vi "Beta.vi"() -> ()   [LabVIEW 2019]
uses:
  Classes/Settings/ObjectSettings/ObjectSettings.lvclass/ObjectSettings.ctl
  <vilib>/Utility/miscctls.llb/LVPositionTypeDef.ctl
  Classes/Parse/ParseVectorFile/ParseVectorFile.lvclass
  C:/Program Files/National Instruments/LabVIEW 2019/vi.lib/JKI/JKI SMO/SMO/SMO.lvclass
  Classes/Settings/Setting Database/Setting Database.lvclass
  Classes/Tool/Tool Data/Tool Data/Tool Data.lvclass
  Classes/Subpanel/Manager/Subpanel.Edit.lvclass
  C:/Users/Albro/Documents/GitHub/AFM-Lithography/lvsrc/Classes/Subpanel/Subpanel.lvclass
  Classes/Render/BigMAQ/BigMAQ.lvclass
  Classes/Selector/Selector.lvclass
  subVIs/AFM API/AFM_Driver_Manager/AFM_Driver_Manager.lvclass
  <userlib>/Levylab/Configuration/Configuration.lvclass
  Classes/Settings/Setting Database/Typedefs/PublicEvents--Setting Database.RectanglesUpdated.ctl
  Classes/Settings/Rectangle Settings/Rectangle Settings.lvclass
  C:/Users/Albro/Documents/GitHub/AFM-Lithography/lvsrc/Classes/Settings/ObjectSettings/ObjectSettings.lvclass
  Classes/Settings/Setting Database/Typedefs/PublicEvents--Setting Database.PathsUpdated.ctl
  Classes/Settings/Path Settings/Path Settings.lvclass
  Classes/Settings/Setting Database/Typedefs/PublicEvents--Setting Database.FunnelsUpdated.ctl
  Classes/Settings/Funnel Settings/Funnel Settings.lvclass
  Classes/Settings/Setting Database/Typedefs/PublicEvents--Setting Database.DotsUpdated.ctl
  Classes/Settings/Dot Settings/Dot Settings.lvclass
  Classes/Parse/ParsePaths/Path.lvclass
  Classes/Parse/Rectangle/Rectangle.lvclass
  Classes/Parse/Image/SVGImage.lvclass
  Classes/Parse/Dot/Dot.lvclass
  <userlib>/Levylab/Relay Box/Typedefs/Resistor--enum.ctl
  Classes/Render/Inset/Inset.lvclass
  Classes/Log/Log.Litho/Log.Litho.lvclass
  Classes/Settings/Setting Database/Typedefs/PrivateEvents--Setting Database.Add To Group.ctl
  Classes/Settings/Setting Database/Typedefs/PrivateEvents--Setting Database.Create New Group.ctl
  Classes/Settings/Setting Database/Typedefs/PrivateEvents--Setting Database.Refresh.ctl
  Classes/Tool/Tool Data/Tool Data/Typedefs/PrivateEvents--Tool Data.Update Objects.ctl
  Classes/Parse/Image/SVGImage.lvclass/SVGImage.ctl
  Classes/Archiver/ArchiveData.ctl
  Controls/Configuration.ctl
  a998b7c0-e198-41fb-897a-9ce541eca358.vi
  <vilib>/Platform/browser.llb/Open URL in Default Browser (string).vi
  <vilib>/Utility/sysdir.llb/Get System Directory.vi
  Classes/Tool/Tool Path/Tool Path.lvclass
  Classes/Tool/Tool Funnel/Tool Funnel.lvclass
  Classes/Tool/Tool Rectangle/Tool Rectangle.lvclass
  Classes/Tool/Tool Dot/Tool Dots.lvclass
  <userlib>/Levylab/Relay Box/Relay-Box.lvclass
  Classes/Subpanel/Subpanel.lvclass
  <vilib>/JKI/JKI SMO/SMO/SMO.lvclass
  Classes/Settings/ObjectSettings/ObjectSettings.lvclass
  Classes/Identity/Identifier.lvclass
  Classes/Archiver/Archivist.lvclass
panel:
  in  "Tab Selectors":T1(radio)
  out "Zoom":string
  in  "Zoom Type":enum32{"Zoom In", "Zoom Out"}(radio)
  in  "Zoom to Fit":bool
  out "Render":T2(plugin-control)
  out "version":string
  out "Ready?":bool
  out "Estimated Time":string
  in  "Run":bool
  in  "Refresh Button":bool
  in  "Done":bool
  in  "Help":bool
  in  "Abort":bool
  in  "Settings":T3(tab)
  in  "Unarchive":bool
  in  "Archive":bool
  out "Status":string
  in  "Inkscape File (.svg)":path caption="Path"
  in  "Background Image":path caption="Path"
  in  "MCLB":i32(listbox) caption="Multicolumn Listbox 2"
  in  "Type:":u16(ring) caption="Ring" items=["Asylum"]
  in  "CopyRender":bool caption="Save"
  in  "Normal Save Path":path caption="Path"
  in  "Save Render":bool caption="Save"
  out "Slow Alert":bool
  in  "Pixellate?":bool
  out "Sizes Match?":bool
  in  "Overwrite?":bool
  in  "Autosave?":bool
  in  "Autosave Path":path caption="Path"
  out "Image Filename":string
  in  "Image Data Range":cluster{sgl, sgl}(slide)={100.0, 0.0} scale=0.0..100.0
  in  "Data Channel":u32 caption="Numeric" max=3
  in  "Inset Editor":bool
  in  "Voltage Color Scale":dbl caption="Numeric 2"
  in  "Hide Labels?":bool
  # "AFM Lithography"
  # "Patterns"
  # "Object Settings"
  # "Atomic Force Microscope Settings"
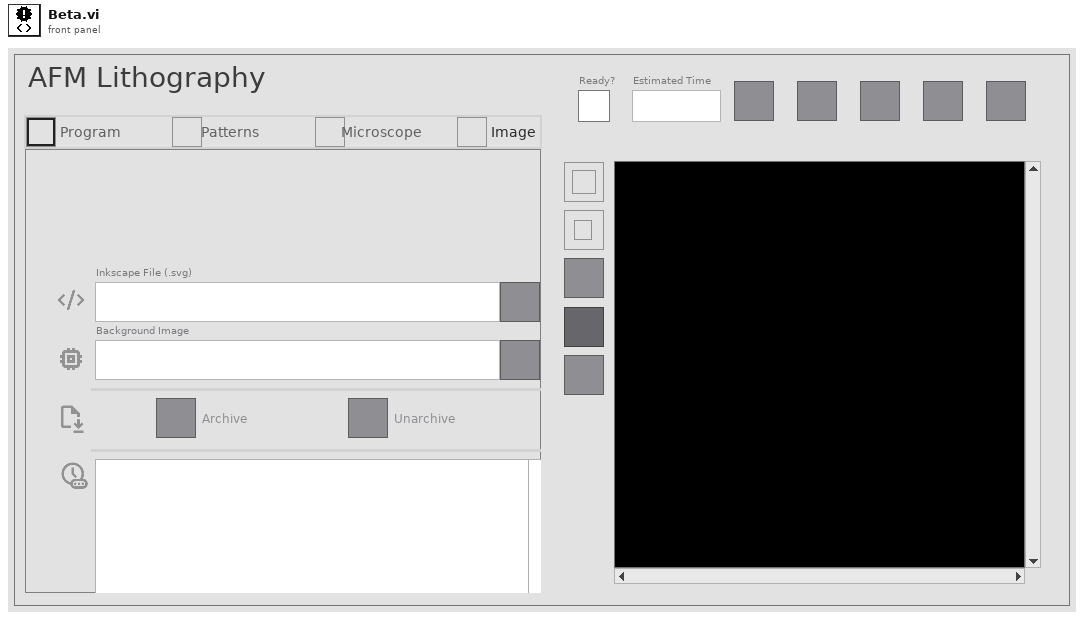
[diagram p1: front panel]
types:
  T1 = enum32{"Home", "Patterns", "Microscope", "Image"}
  T2 = typedef "IMAQ Image.ctl" = refnum<image>
  T3 = enum32{"Program Settings", "Patterns and Writing", "AFM Settings", "Image Settings"}
  T4 = cluster{"Groups":string[], "Enable Items":bool[]}
  T5 = typedef "LVPositionTypeDef.ctl" = cluster{"Left":i32, "Top":i32}
  T6 = cluster{"Point":T5, "Button":u16, "PlatMods":cluster{"Shift":bool, "Ctrl":bool, "Alt":bool, "Cmd":bool, "Opt":bool}}
  T7 = enum32{"Invalid", "Standard", "Closed", "Hidden", "Minimized", "Maximized"}
  T8 = enum32{"invalid app kind", "Development System", "Run Time System", "Student Edition", "Embedded LabVIEW", "Evaluation", "Custom"}
  T9 = cluster{"Background.Range":cluster{sgl, sgl}, "Background.Page":i32}
  T10 = enum8{"Enabled", "Disabled", "Disabled and Grayed Out"}
  T11 = cluster{"Pattern":string, "Pattern Label":string, "Prompt":string}
  T12 = cluster{"paths":string[], "funnels":string[], "rects":string[], "dots":string[]}
  T13 = typedef "Setting Database.lvclass/PrivateEvents--Setting Database.Add To Group.ctl" = cluster{"Name":string, "Group":string}
  T14 = typedef "Setting Database.lvclass/PrivateEvents--Setting Database.Create New Group.ctl" = cluster{"Name":string, "Group":string}
  T15 = typedef "Setting Database.lvclass/PrivateEvents--Setting Database.Refresh.ctl" = cluster{"Paths":string[], "Rectangles":string[], "Funnels":string[], "Dots":string[]}
  T16 = cluster{"Paths":refnum<class "Path.lvclass">[], "Rectangles":refnum<class "Rectangle.lvclass">[], "SVGImage":refnum<class "SVGImage.lvclass">, "Dots":refnum<class "Dot.lvclass">[], "Funnels":refnum<class "Path.lvclass">[]}
  T17 = typedef "Tool Data.lvclass/PrivateEvents--Tool Data.Update Objects.ctl" = cluster{"Settings":cluster{"Paths":T18, "Rectangles":T19, "Funnels":T20, "Dots":T21}, "Data":cluster{"Paths":refnum<class "Path.lvclass">[], "Rectangles":refnum<class "Rectangle.lvclass">[], "SVGImage":refnum<class "SVGImage.lvclass">, "Dots":refnum<class "Dot.lvclass">[], "Funnels":refnum<class "Path.lvclass">[]}}
  T18 = typedef "Setting Database.lvclass/PublicEvents--Setting Database.PathsUpdated.ctl" = refnum<class "Path Settings.lvclass">[]
  T19 = typedef "Setting Database.lvclass/PublicEvents--Setting Database.RectanglesUpdated.ctl" = refnum<class "Rectangle Settings.lvclass">[]
  T20 = typedef "Setting Database.lvclass/PublicEvents--Setting Database.FunnelsUpdated.ctl" = refnum<class "Funnel Settings.lvclass">[]
  T21 = typedef "Setting Database.lvclass/PublicEvents--Setting Database.DotsUpdated.ctl" = refnum<class "Dot Settings.lvclass">[]
  T22 = typedef "Archivist.lvclass/ArchiveData.ctl" = cluster{"Settings":cluster{"Paths":T18, "Rectangles":T19, "Funnels":T20, "Dots":T21}, "Data Files":cluster{"svg":path, "afm":path, "jpg":path}, "Input Path":path, "Order":string[]}
  T23 = typedef "Configuration.ctl" = cluster{"Inkscape Path":path, "Background Path":path, "Autosave Render Path":path, "Autosave Render":bool, "Hide Labels":bool, "Normal Render Path":path, "Overwrite":bool}
  T24 = typedef "Relay-Box.lvclass/Resistor--enum.ctl" = enum16{"open", "discharge tip", "0 ohms", "100k ohm", "10M ohm", "1G ohm"}
  T25 = cluster{"Core":cluster{"Current VI Reference":refnum<vi>, "Close Panel on Exit?":bool}, "tooler":refnum<class "Tool Data.lvclass">, "parser":refnum<class "ParseVectorFile.lvclass">, "settings":refnum<class "Setting Database.lvclass">, "selector":refnum<class "Selector.lvclass">, "sbpnl.edit":refnum<class "Subpanel.Edit.lvclass">, "big-maq":refnum<class "BigMAQ.lvclass">, "config":refnum<class "Configuration.lvclass">, "afm_mngr":refnum<class "AFM_Driver_Manager.lvclass">, "Obj Settings":cluster{"Rectangles":T19, "Paths":T18, "Funnels":T20, "Dots":T21}, "Changed Obj":cluster{"Path Changes":cluster{bool, "index of element":i32}[], "Funnel Changes":cluster{bool, "index of element":i32}[], "Rectangle Changes":cluster{bool, "index of element":i32}[], "Dot Changes":cluster{bool, "index of element":i32}[]}, "GUIDs":cluster{"Dots":string[], "Funnels":string[], "Rects":string[], "Paths":string[]}, "Parsed Obj":cluster{"Paths":refnum<class "Path.lvclass">[], "Rectangles":refnum<class "Rectangle.lvclass">[], "Background":refnum<class "SVGImage.lvclass">, "Dots":refnum<class "Dot.lvclass">[], "Funnels":refnum<class "Path.lvclass">[], "Other Images":refnum<class "SVGImage.lvclass">[]}, "Litho":cluster{"Name":string, "Litho":cluster{"X":dbl, "Y":dbl, "Speed":dbl, "Voltage":dbl}[], "Set Resistance":T24, "Meta":variant}[], "root path":path, "UI":cluster{"Hide Labels":bool, "Image Data Range":cluster{sgl, sgl}, "Status":string, "Autosave Path":path, "Autosave?":bool, "Inkscape File (.svg)":path, "Background Image":path, "Page":u32, "Normal Save Path":path, "Overwrite":bool, "Pixellate?":bool}, "inset":refnum<class "Inset.lvclass">, "log":refnum<class "Log.Litho.lvclass">, "Offline Log":string, "Zoom History":cluster{"X":sgl, "Y":sgl}[], "Archive Location":path, "Cancel Archive":bool}
  T26 = typedef "LVPoint32TypeDef.ctl" = cluster{"Horizontal":i32, "Vertical":i32}
  T27 = cluster{"Paths":refnum<class "Tool Path.lvclass">[], "Funnels":refnum<class "Tool Funnel.lvclass">[], "Rectangles":refnum<class "Tool Rectangle.lvclass">[], "Dots":refnum<class "Tool Dots.lvclass">[]}
  T28 = cluster{"Shift":bool, "Ctrl":bool, "Alt":bool, "Cmd":bool, "Opt":bool}
  T29 = cluster{"Hide Labels":bool, "Image Data Range":cluster{sgl, sgl}, "Status":string, "Autosave Path":path, "Autosave?":bool, "Inkscape File (.svg)":path, "Background Image":path, "Page":u32, "Normal Save Path":path, "Overwrite":bool, "Pixellate?":bool}
  T30 = cluster{"Name":string, "Litho":cluster{"X":dbl, "Y":dbl, "Speed":dbl, "Voltage":dbl}[], "Set Resistance":T24, "Meta":variant}[]
  T31 = cluster{"Paths":refnum<class "Path.lvclass">[], "Rectangles":refnum<class "Rectangle.lvclass">[], "Background":refnum<class "SVGImage.lvclass">, "Dots":refnum<class "Dot.lvclass">[], "Funnels":refnum<class "Path.lvclass">[], "Other Images":refnum<class "SVGImage.lvclass">[]}
  T32 = cluster{"Dots":string[], "Funnels":string[], "Rects":string[], "Paths":string[]}
  T33 = cluster{"Path Changes":cluster{bool, "index of element":i32}[], "Funnel Changes":cluster{bool, "index of element":i32}[], "Rectangle Changes":cluster{bool, "index of element":i32}[], "Dot Changes":cluster{bool, "index of element":i32}[]}
  T34 = cluster{"Rectangles":T19, "Paths":T18, "Funnels":T20, "Dots":T21}
  T35 = cluster{"Current VI Reference":refnum<vi>, "Close Panel on Exit?":bool}
  T36 = typedef "AFM_Driver_Manager.lvclass/AFM_Driver_Manager.PublicEvents.ctl" = cluster{"Lithography Done":refnum<user-event>}
  T37 = typedef "Setting Database.lvclass/PublicEvents--Cluster.ctl" = cluster{"NewActivePath":refnum<user-event>, "PathsUpdated":refnum<user-event>, "RectanglesUpdated":refnum<user-event>, "NewActiveRectangle":refnum<user-event>, "NewActiveFunnel":refnum<user-event>, "FunnelsUpdated":refnum<user-event>, "NewActiveDot":refnum<user-event>, "DotsUpdated":refnum<user-event>}
  T38 = typedef "ParseVectorFile.lvclass/PublicEvents--Cluster.ctl" = cluster{"ParsedData":refnum<user-event>}
  T39 = typedef "Tool Data.lvclass/PublicEvents--Cluster.ctl" = cluster{"Objects Updated":refnum<user-event>}
  T40 = typedef "SMO.lvclass/SMOState --Enum.ctl" = enum16{"unknown", "Created", "Started", "Stopped"}
  T41 = typedef "Selector.lvclass/Item.ctl" = cluster{"Name":string, "Group":string, "Enabled":bool}
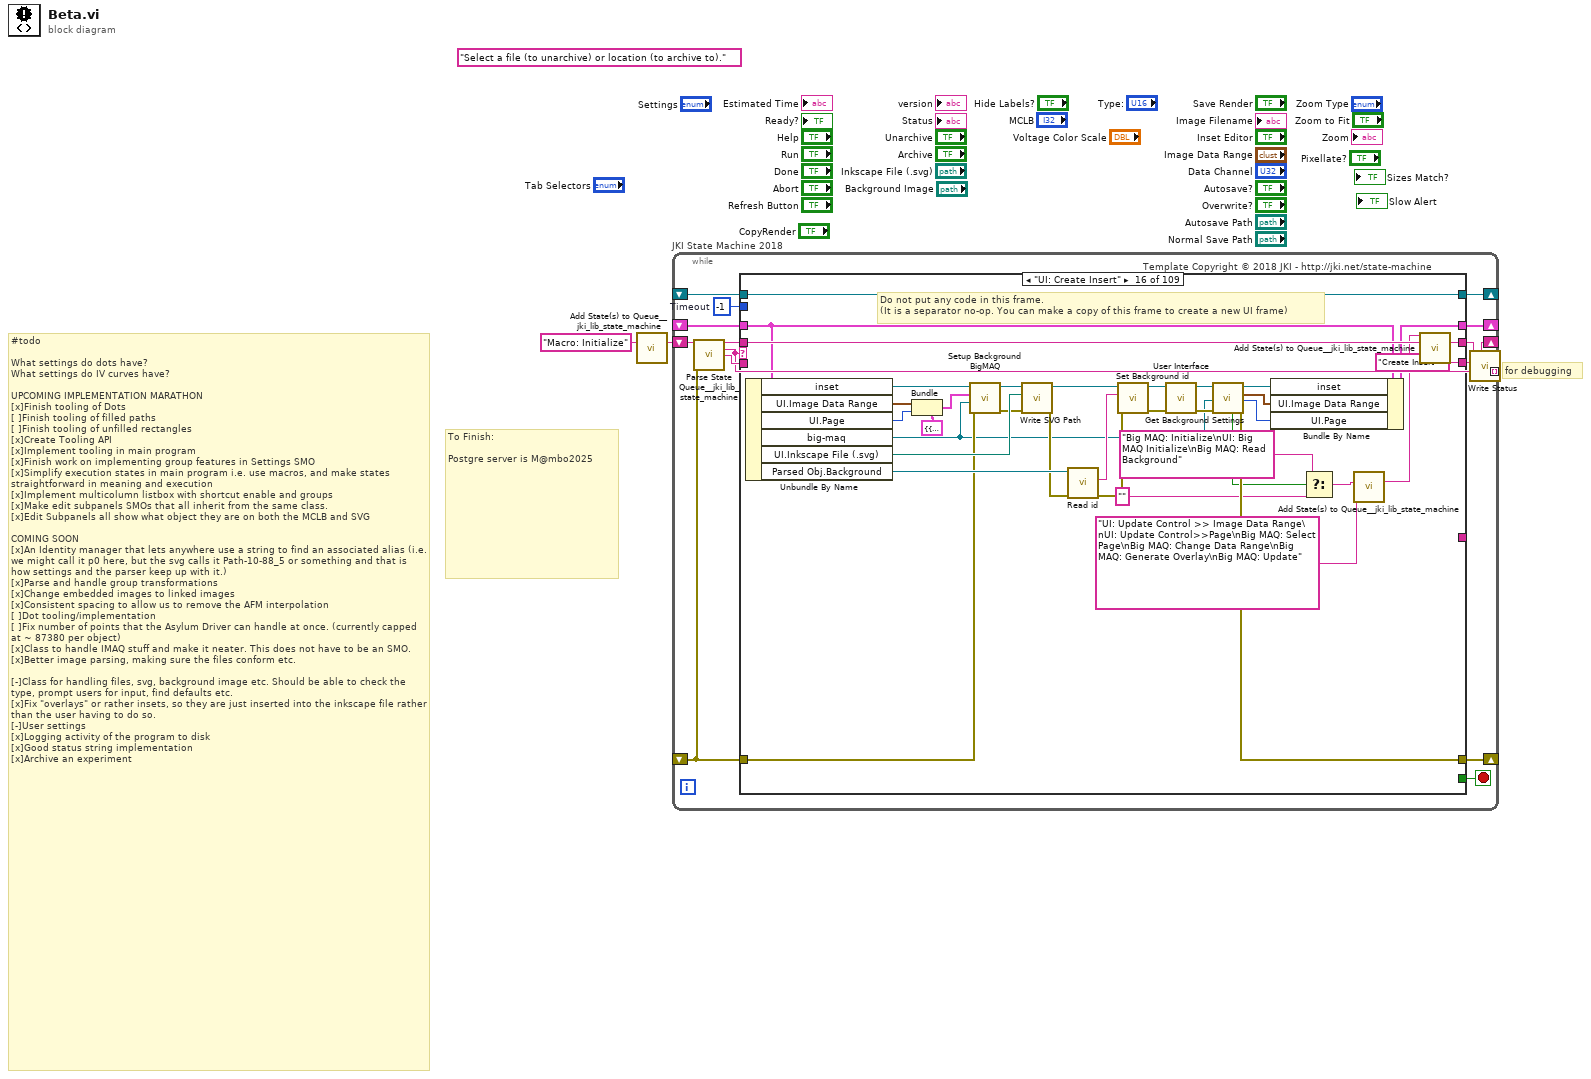
[diagram p0: block diagram]
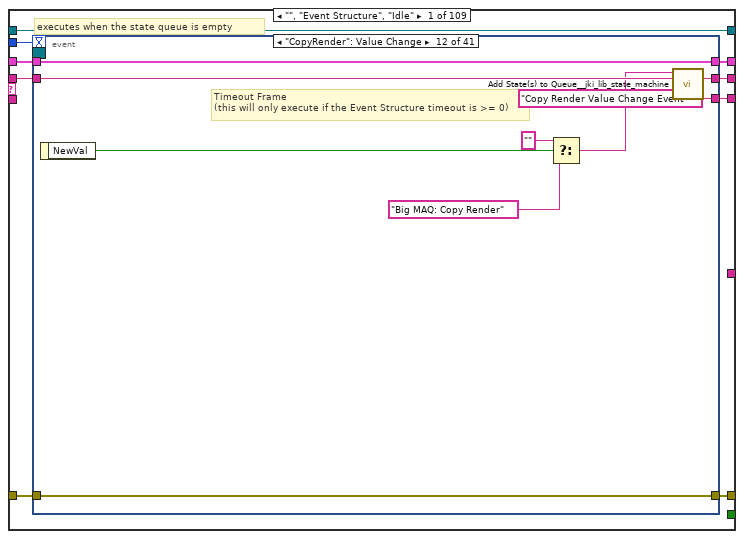
[diagram p2: hidden frame]
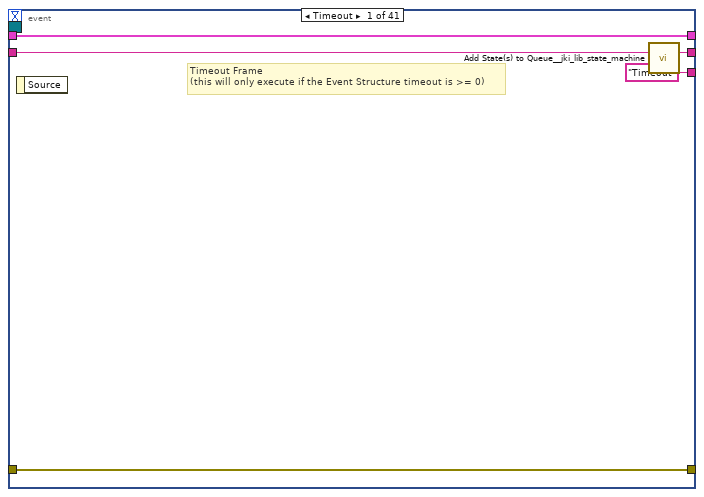
[diagram p3: hidden frame]
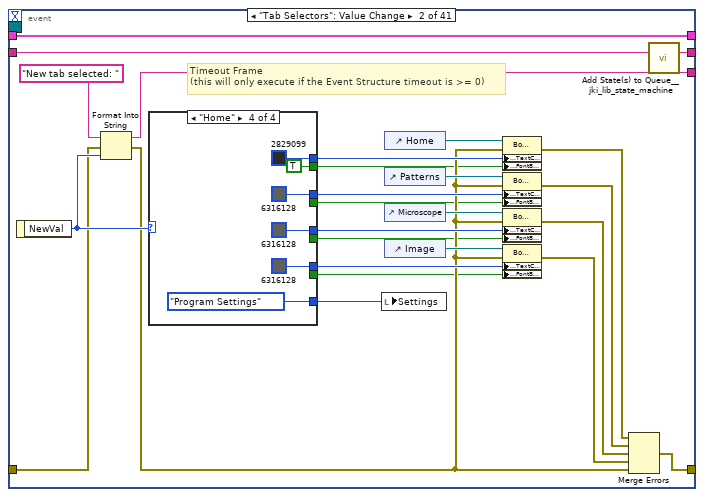
[diagram p4: hidden frame]
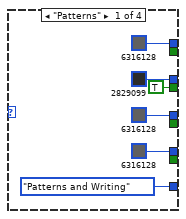
[diagram p5: hidden frame]
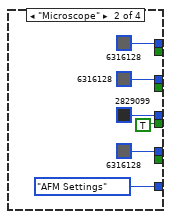
[diagram p6: hidden frame]
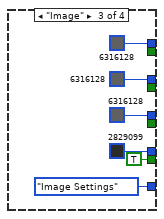
[diagram p7: hidden frame]
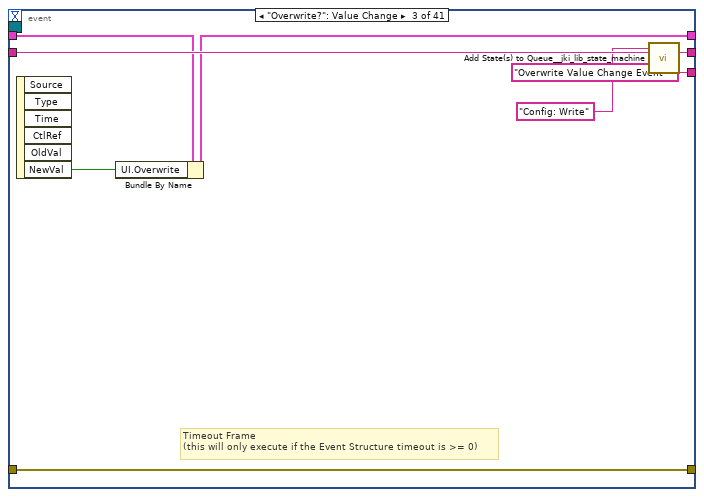
[diagram p8: hidden frame]
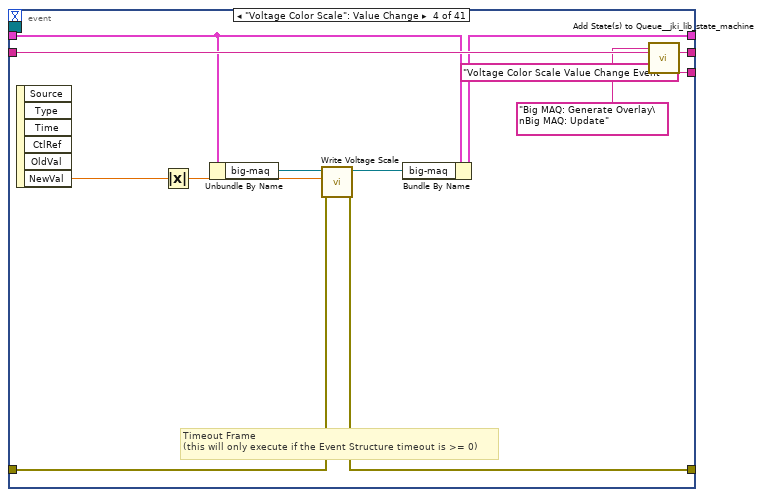
[diagram p9: hidden frame]
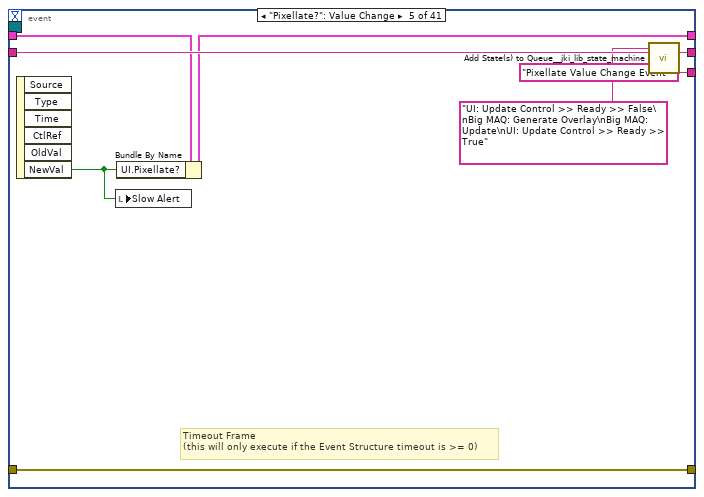
[diagram p10: hidden frame]
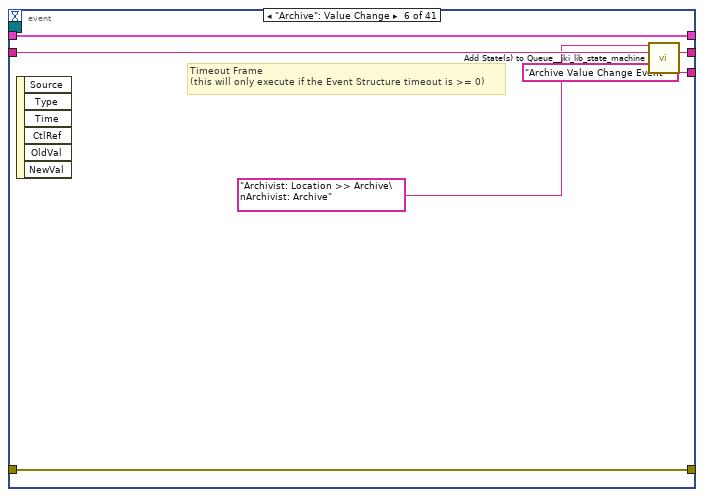
[diagram p11: hidden frame]
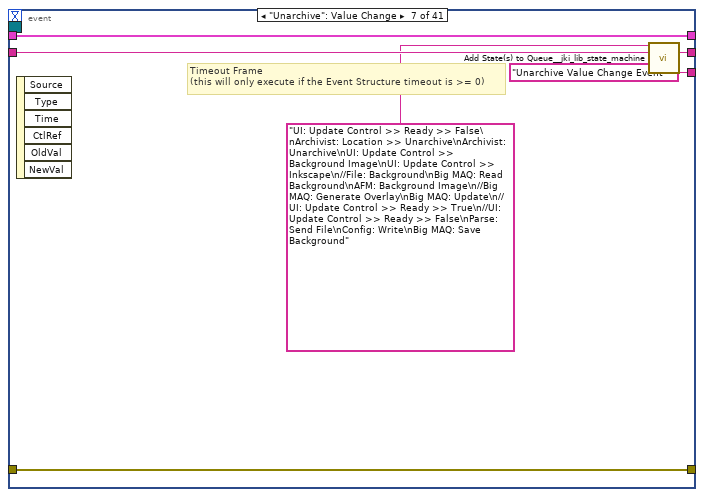
[diagram p12: hidden frame]
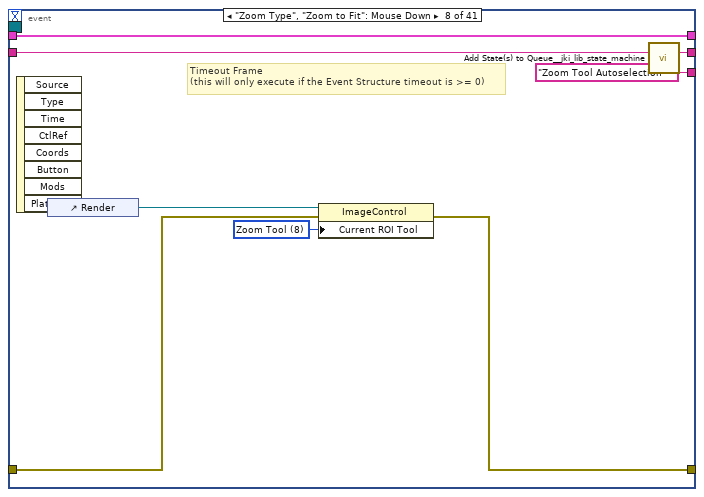
[diagram p13: hidden frame]
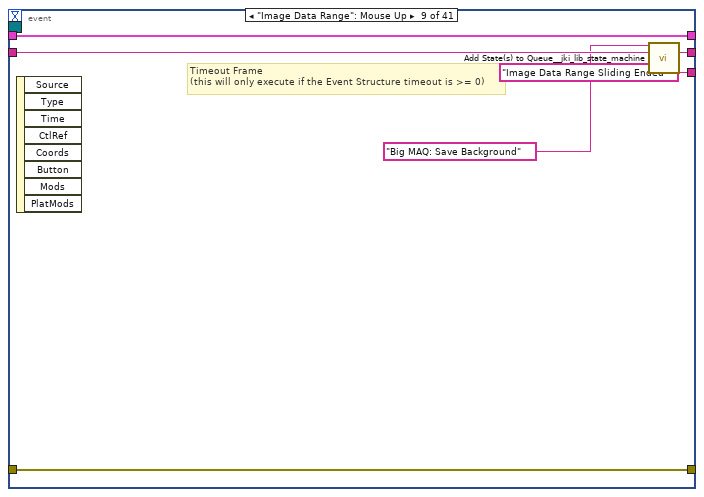
[diagram p14: hidden frame]
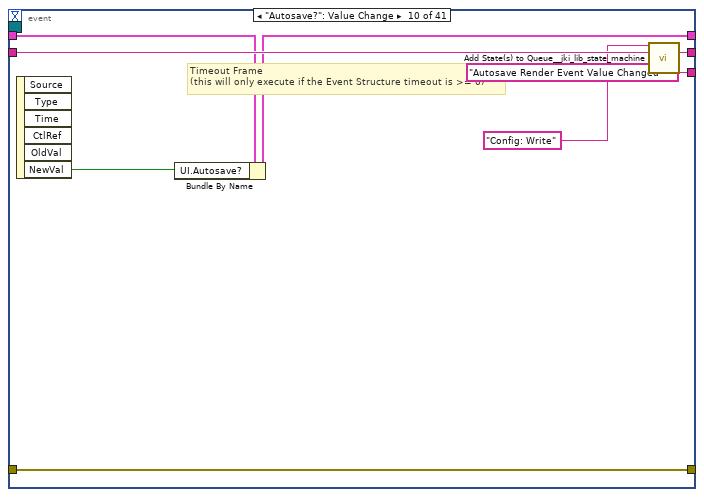
[diagram p15: hidden frame]
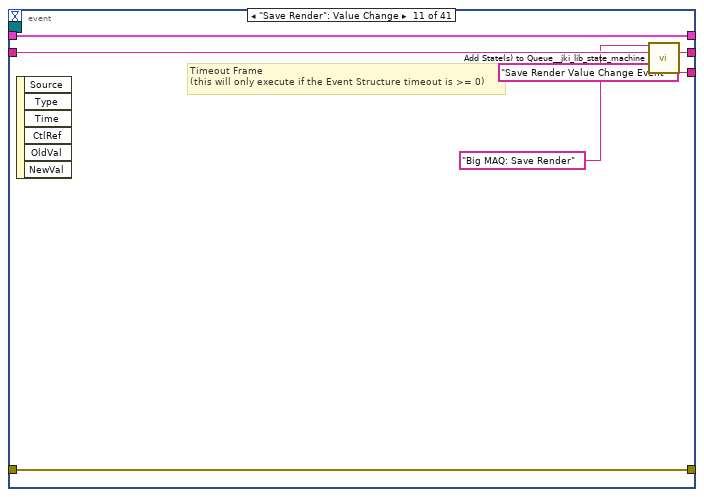
[diagram p16: hidden frame]
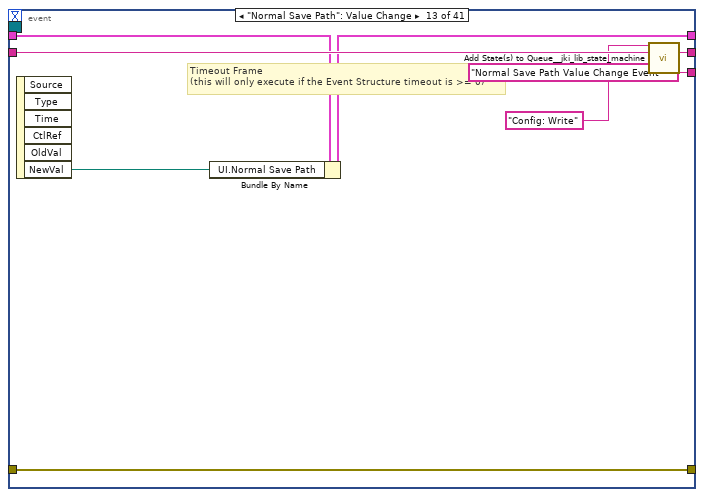
[diagram p17: hidden frame]
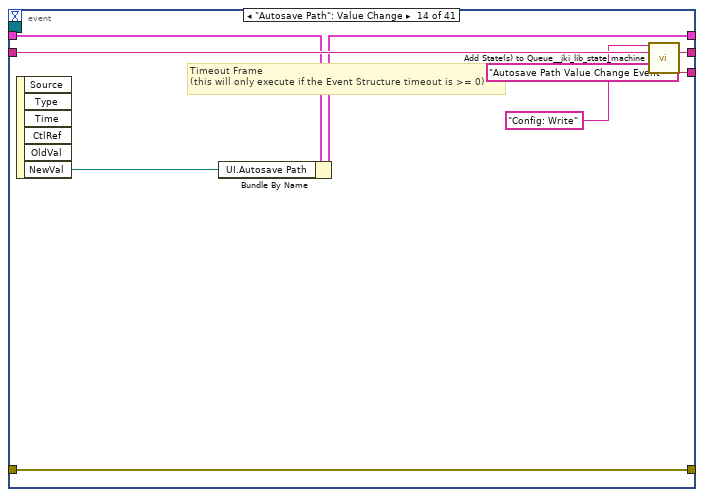
[diagram p18: hidden frame]
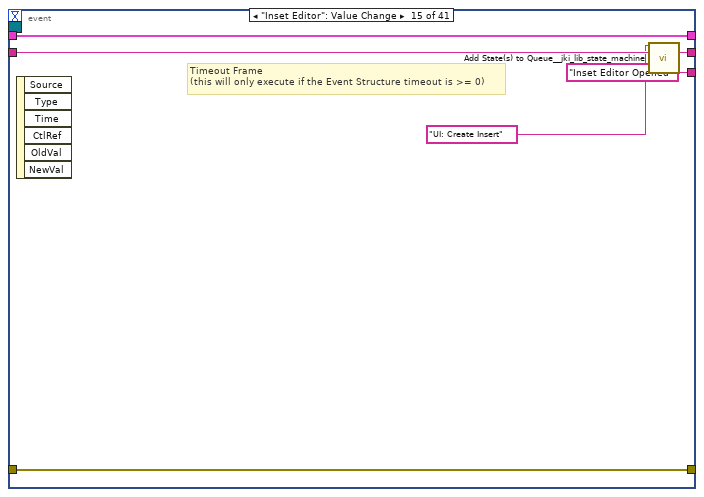
[diagram p19: hidden frame]
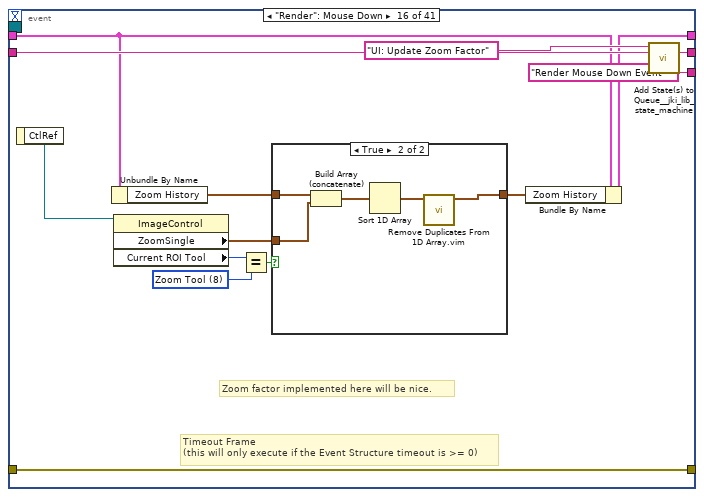
[diagram p20: hidden frame]
diagram:
  (unwired) "Select a file (to unarchive) or location (to archive to)." ("prompt")
  # "for debugging"
  # "#todo\n\nWhat settings do dots have?\nWhat settings do IV curves have?\n\nUPCOMING IMPLEMENTATION MARATHON\n[x]Finish tooling of Dots\n[ ]Finish tooling of filled paths\n[ ]Finish tooling of unfilled rectangles\n[x]Create Tooling API\n[x]Implement tooling in main program\n[x]Finish work on implementing group features in Settings SMO\n[x]Simplify execution states in main program i.e. use macros, and make states straightforward in meaning and execution\n[x]Implement multicolumn listbox with shortcut enable and groups\n[x]Make edit subpanels SMOs that all inherit from the same class.\n[x]Edit Subpanels all show what object they are on both the MCLB and SVG\n\nCOMING SOON\n[x]An Identity manager that lets anywhere use a string to find an associated alias (i.e. we might call it p0 here, but the svg calls it Path-10-88_5 or something and that is how settings and the parser keep up with it.)\n[x]Parse and handle group transformations\n[x]Change embedded images to linked images\n[x]Consistent spacing to allow us to remove the AFM interpolation\n[ ]Dot tooling/implementation\n[ ]Fix number of points that the Asylum Driver can handle at once. (currently capped at ~ 87380 per object)\n[x]Class to handle IMAQ stuff and make it neater. This does not have to be an SMO.\n[x]Better image parsing, making sure the files conform etc.\n\n[-]Class for handling files, svg, background image etc. Should be able to check the type, prompt users for input, find defaults etc.\n[x]Fix \"overlays\" or rather insets, so they are just inserted into the inkscape file rather than the user having to do so.\n[-]User settings\n[x]Logging activity of the program to disk\n[x]Good status string implementation\n[x]Archive an experiment"
  # "To Finish:\n\nPostgre server is M@mbo2025"
  n1 = call <vilib>:"Add State(s) to Queue__jki_lib_state_machine.vi"("State(s) in (\"\")"="Macro: Initialize") -> ("States Out"=w2:string)  [unwired: 14 in]
  n2 = while "JKI State Machine 2018" {
    shift-right: [w12] -> _
    shift-left: _ -> [w11]
    shift-right: [w14] -> _
    shift-left: _ -> [w9]
    shift-right: [w4] -> _
    shift-left: w2 -> [w15]
    shift-right: [w8] -> _
    shift-left: _ -> [w7]
    tunnel: [w3] -> _ mode=indexing
    stop <- w13 stop-if-true
    w10 = -1  # Timeout
    # "Template Copyright © 2018 JKI - http://jki.net/state-machine"
    n3 = call <vilib>:"Parse State Queue__jki_lib_state_machine.vi"("State Queue"=w15, "Error In (no error)"=w9) -> ("Remaining States"=w17:string, "Current State"=w3:string, "Arguments"=w16:string)  [unwired: 11 in]
    n4 = case shown="\"UI: Create Insert\"" w3 {
      selector: w3 -> [_ _ w577 _ _ _ _ _ _ _ _ _ _ _ _ _ _ _ _ _ _ _ _ _ _ _ _ _ _ _ _ _ _ _ _ _ _ _ _ _ _ _ _ _ _ _ _ _ _ _ _ _ _ _ _ _ _ _ _ _ _ _ _ _ _ _ _ _ _ _ _ _ _ _ _ _ _ _ _ _ _ _ _ _ _ _ _ _ _ _ _ _ _ _ _ _ _ _ _ _ _ _ _ _ _ _ _ _ _]
      tunnel: w17 -> [w26 w574 w581 w602 w623 w629 w634 w641 w673 w680 w685 w705 w712 w717 w737 w799 w812 w822 w837 w854 w878 w886 w981 w998 w1010 w1080 w1086 w1092 w1098 w1104 w1110 w1121 w1126 w1135 w1143 w1148 w1167 w1198 w1210 w1217 w1232 w1239 w1250 w1262 w1274 w1281 w1296 w1334 w1352 w1391 w1403 w1418 w1425 w1443 w1466 w1480 w1503 w1516 w1528 w1535 w1556 w1579 w1591 w1601 w1615 w1631 w1646 w1659 w1671 w1683 w1693 w1713 w1731 w1746 w1753 w1770 w1798 w1808 w1818 w1835 w1845 w1861 w1887 w1923 w1930 w1942 w1952 w1964 w1969 w1987 w2022 w2063 w2094 w2107 w2120 w2127 w2139 w2158 w2179 w2186 w2196 w2206 w2217 w2228 w2238 w2249 w2261 w2275 w2285]
      tunnel: w16 -> [_ _ _ _ _ _ _ _ _ _ _ _ _ _ _ _ _ _ w826 w838 _ w881 _ w993 w1004 _ _ _ _ _ _ _ _ _ _ _ _ _ _ _ _ _ _ _ _ _ w1285 w1327 w1344 _ _ _ _ _ _ _ _ _ _ _ _ w1572 _ _ _ _ _ _ _ _ _ _ _ _ _ w1754 _ _ _ w1827 _ _ w1879 _ _ w1933 _ _ _ w1977 _ _ _ _ _ _ _ _ _ _ _ _ _ _ _ _ w2252 _ _]
      tunnel: w11 -> [w24 w571 w579 w595 w620 w627 w631 w639 _ w675 w682 w701 w710 w714 w734 w794 w801 w816 w835 w849 w873 w889 w974 w996 w1006 w1077 w1083 w1089 w1095 w1101 w1107 w1118 w1123 w1130 w1136 w1145 w1152 w1189 w1207 w1215 w1226 w1235 w1247 w1259 w1271 w1277 w1293 w1331 w1349 w1388 w1400 w1415 w1421 w1440 w1457 w1477 w1500 w1513 w1525 w1531 w1553 w1576 w1588 w1598 w1612 w1628 w1643 w1656 w1668 w1680 w1690 w1710 w1728 w1743 w1749 w1755 w1795 w1805 w1815 w1832 w1842 w1858 w1884 w1920 w1926 w1939 w1949 w1961 w1965 w1978 w2015 w2054 w2090 w2104 w2117 w2123 w2136 w2152 w2176 w2182 w2193 w2203 w2214 w2225 w2235 w2246 w2258 w2272 w2282]
      tunnel: [w23 w572 w583 w599 errorcluster {"status"=FALSE, "code"=0, "source"=""} ("error out") w626 w632 w636 w670 w676 w683 w697 w707 w715 w735 w774 w810 w818 w825 w844 w867 w885 w962 w994 w1007 w1078 w1084 w1090 w1096 w1102 w1108 w1119 w1124 w1133 w1141 w1146 w1158 w1181 w1208 w1213 w1229 w1237 w1242 w1253 w1265 w1279 w1287 w1326 w1337 w1377 w1393 w1409 w1423 w1428 w1462 w1473 w1487 w1508 w1519 w1533 w1546 w1569 w1585 w1595 w1609 w1620 w1640 w1652 w1664 w1677 w1684 w1707 w1725 w1733 w1751 w1761 w1790 w1801 w1811 w1826 w1838 w1853 w1881 w1918 w1928 w1936 w1946 w1956 w1967 w1971 w2014 w2056 w2092 w2098 w2112 w2125 w2130 w2151 w2170 w2184 w2189 w2200 w2210 w2218 w2231 w2242 w2254 w2265 w2278] -> w14
      tunnel: w9 -> [w22 w572 w582 w599 w617 w626 w632 w637 w670 w677 w683 w690 w708 w715 w735 w778 w810 w817 w824 w847 w872 w883 w975 w995 w1008 w1078 w1084 w1090 w1096 w1102 w1108 w1119 w1124 w1133 w1141 w1146 w1157 w1188 w1208 w1212 w1228 w1237 w1241 w1252 w1264 w1279 w1282 w1325 w1336 w1378 w1394 w1406 w1423 w1427 w1458 w1472 w1486 w1507 w1518 w1533 w1548 w1568 w1584 w1594 w1608 w1619 w1639 w1651 w1660 w1676 w1685 w1706 w1724 w1741 w1751 w1760 w1789 w1800 w1810 w1825 w1839 w1852 w1880 w1917 w1928 w1935 w1945 w1957 w1967 w1984 w2013 w2055 w2092 w2097 w2111 w2125 w2129 w2150 w2169 w2184 w2188 w2199 w2209 w2219 w2230 w2241 w2253 w2264 w2277]
      tunnel: [w25 w573 w580 w601 w622 w628 w633 w640 w672 w679 w684 w704 w711 w716 w736 w798 w811 w821 w836 w853 w877 w890 w980 w997 w1009 w1079 w1085 w1091 w1097 w1103 w1109 w1120 w1125 w1134 w1142 w1147 w1166 w1197 w1209 w1216 w1231 w1238 w1249 w1261 w1273 w1280 w1295 w1333 w1351 w1390 w1402 w1417 w1424 w1442 w1465 w1479 w1502 w1515 w1527 w1534 w1555 w1578 w1590 w1600 w1614 w1630 w1645 w1658 w1670 w1682 w1692 w1712 w1730 w1745 w1752 w1769 w1797 w1807 w1817 w1834 w1844 w1860 w1886 w1922 w1929 w1941 w1951 w1963 w1968 w1986 w2021 w2062 w2093 w2106 w2119 w2126 w2138 w2157 w2178 w2185 w2195 w2205 w2216 w2227 w2237 w2248 w2260 w2274 w2284] -> w6
      tunnel: [_ _ _ _ _ TRUE _ _ _ _ _ _ _ _ _ _ _ _ _ _ _ _ _ _ _ _ _ _ _ _ _ _ _ _ _ _ _ _ _ _ _ _ _ _ _ _ _ _ _ _ _ _ _ _ _ _ _ _ _ _ _ _ _ _ _ _ _ _ _ _ _ _ _ _ _ _ _ _ _ _ _ _ _ _ _ _ _ _ _ _ _ _ _ _ _ _ _ _ _ _ _ _ _ _ _ _ _ _ _] -> w13
      tunnel: [w21 w571 w579 w600 w620 w627 w631 w639 w671 w675 w682 w701 w710 w714 w734 w795 w801 w819 w835 w851 w874 w888 w974 w996 w1006 w1077 w1083 w1089 w1095 w1101 w1107 w1118 w1123 w1131 w1137 w1145 w1153 w1190 w1207 w1215 w1226 w1236 w1248 w1260 w1272 w1278 w1294 w1332 w1350 w1389 w1401 w1416 w1422 w1441 w1464 w1478 w1501 w1514 w1526 w1532 w1554 w1577 w1589 w1599 w1613 w1629 w1644 w1657 w1669 w1681 w1691 w1711 w1729 w1744 w1750 w1768 w1796 w1806 w1816 w1833 w1843 w1859 w1885 w1921 w1927 w1940 w1950 w1962 w1965 w1982 w2016 w2054 w2091 w2105 w2118 w2124 w2137 w2156 w2177 w2183 w2194 w2204 w2215 w2226 w2236 w2247 w2259 w2273 w2283] -> w12
      tunnel: w10 -> [w20 _ _ _ _ _ _ _ _ _ _ _ _ _ _ _ _ _ _ _ _ _ _ _ _ _ _ _ _ _ _ _ _ _ _ _ _ _ _ _ _ _ _ _ _ _ _ _ _ _ _ _ _ _ _ _ _ _ _ _ _ _ _ _ _ _ _ _ _ _ _ _ _ _ _ _ _ _ _ _ _ _ _ _ _ _ _ _ _ _ _ _ _ _ _ _ _ _ _ _ _ _ _ _ _ _ _ _ _]
      tunnel: [w19 w570 w576 w589 w618 w624 w630 w638 w655 w674 w681 w703 w709 w713 w733 w797 w809 w820 w834 w852 w876 w884 w979 w992 w1003 w1076 w1082 w1088 w1094 w1100 w1105 w1111 w1122 w1132 w1140 w1144 w1165 w1196 w1206 w1214 w1230 w1233 w1246 w1258 w1270 w1275 w1292 w1330 w1348 w1387 w1399 w1414 w1419 w1439 w1463 w1476 w1499 w1512 w1524 w1529 w1552 w1575 w1583 w1593 w1605 w1617 w1633 w1650 w1667 w1675 w1689 w1705 w1723 w1740 w1747 w1767 w1794 w1804 w1814 w1824 w1837 w1847 w1878 w1915 w1924 w1932 w1944 w1954 w1966 w1985 w2020 w2061 w2088 w2103 w2116 w2121 w2135 w2155 w2175 w2180 w2192 w2202 w2213 w2224 w2234 w2245 w2257 w2271 w2281] -> w8
      tunnel: w7 -> [w19 w570 w576 w589 w618 w624 w630 w638 w655 w674 w681 _ w709 w713 w733 w797 w809 w820 w834 w852 w876 w884 w979 w992 w1003 w1076 w1082 w1088 w1094 w1100 w1105 w1111 w1122 w1132 w1140 w1144 w1165 w1196 w1206 w1214 w1230 w1233 w1246 w1258 w1270 w1275 w1292 w1330 w1348 w1387 w1399 w1414 w1419 w1439 w1463 w1476 w1499 w1512 w1524 w1529 w1552 w1575 w1583 w1593 w1605 w1617 w1633 w1650 w1667 w1675 w1689 w1705 w1723 w1740 w1747 w1767 w1794 w1804 w1814 w1824 w1837 w1847 w1878 w1915 w1924 w1932 w1944 w1954 w1966 w1985 w2020 w2061 w2088 w2103 w2116 w2121 w2135 w2155 w2175 w2180 w2192 w2202 w2213 w2224 w2234 w2245 w2257 w2271 w2281]
      tunnel: [w18 _ "Default State Encountered??" ("t") "" w611 _ _ "Status Log Setup" "" _ _ "Events registered" "Events Unregistered" _ "Initialize the Fancy Tab Control UI" ("t") "Create Insert" "Update Zoom Factor Display" "Select Initialization" "Run Enable/Disabled" "" "Big-MAQ Control UI Initialized" w879 "UI Initialization" _ _ _ _ _ _ _ _ _ _ _ _ _ _ _ _ "Identity registry disposed" "Identity Registry Populated" _ "Inkscape File Sent to Parser" "Parser Stopped" "Parser Started" _ "New Active Object -- Settings Database" "Object Enabled State Changed" "Object Group Association Changed -- Sent to Settings Database" "Refresh Settings Database" "Settings Database Stopped" "Settings Database Started" _ "Tooler: Paths Sorted" "Tooler: Object IDs Determined" "Tooler generated Lithography Data" "Data Sent to Tooler" "Tooler Stopped" "Tooler started" _ w1542 "Big MAQ show-hide labels executed" "Big MAQ Zoom to Fit Executed" "Big-MAQ control updated" "Overlay Generated" "New Image Page Selected" "Image Data Range Updated" "Big MAQ Read Background" "Background for inkscape file save." ("t") "Render Saved to Disk" "Render Copied to Clipboard" w1701 "Big-MAQ Closed Down" "Big-MAQ IMAQ manager Initialized" _ "Selector value changed by name." ("t") "New population of values inserted into selector." ("t") "Selector Updated" "Checkmarks applied" "Selector Model Value Changed" "Selector Model Order Updated" "Lithography Data Ordered" "Object Group Association Changed" "Selector Created" _ "New Property Subpanel Inserted" "Subpanel Closed" "Properties Subpanel Initialized" _ w1973 "Unarchiving File" ("t") "State saved to archive" ("t") _ "Logger started" "Logger Stopped" _ "Configuration Initialized" "Configuration Written" "Configuration Read" _ "Lithography process finished." "AFM Manager Stopped" "Background Image Sent to Driver" "Lithography Data Sent to Driver" "Run Lithography Message Sent" "AFM Driver Inserted Into Subpanel" "Active AFM Driver Set" "AFM Driver Launched and Initialized" "AFM Driver Manager Initialized"] -> w5
      tunnel: [_ _ _ _ w611 _ _ _ _ _ _ _ _ _ _ _ _ _ _ _ _ _ _ _ _ _ _ _ _ _ _ _ _ _ _ _ _ _ _ _ _ _ _ _ _ _ _ _ _ _ _ _ _ _ _ _ _ _ _ _ _ _ _ _ _ _ _ _ _ _ _ _ _ _ _ _ _ _ _ _ _ _ _ _ _ _ _ _ _ _ _ _ _ _ _ _ _ _ _ _ _ _ _ _ _ _ _ _ _] -> _
      frame "", "Event Structure", "Idle" {
        # "executes when the state queue is empty"
        n5 = event shown="[11] \"CopyRender\": Value Change" {
          selector: w19 -> [_ _ _ _ _ _ _ _ _ _ _ _ _ _ _ _ _ _ _ _ _ _ _ _ _ _ _ _ _ _ _ _ _ _ _ _ _ _ _ _ _]
          dyn-events: _ -> [_ _ _ _ _ _ _ _ _ _ _ _ _ _ _ _ _ _ _ _ _ _ _ _ _ _ _ _ _ _ _ _ _ _ _ _ _ _ _ _ _]
          timeout: w20 -> [_ _ _ _ _ _ _ _ _ _ _ _ _ _ _ _ _ _ _ _ _ _ _ _ _ _ _ _ _ _ _ _ _ _ _ _ _ _ _ _ _]
          tunnel: w26 -> [w31 w57 w89 w101 w109 w115 w121 w129 w135 w143 w149 w158 w166 w174 w180 w194 w217 w224 w235 w241 w247 w253 w261 w269 w277 w285 w291 w304 w310 w334 w371 w408 w445 w474 w486 w501 w521 w531 w542 w555 w561]
          tunnel: [w30 w56 w88 w100 w108 w114 w120 w128 w134 w142 w148 w157 w165 w173 w179 w193 w216 w223 w234 w240 w246 w252 w260 w268 w276 w284 w290 w303 w309 w333 w370 w407 w444 w473 w485 w500 w520 w530 w541 w554 w560] -> w25
          tunnel: w24 -> [w28 w55 w84 w96 w104 w112 w118 w127 w132 w138 w146 w155 w161 w169 w177 w181 w206 w222 w226 w238 w244 w249 w256 w264 w272 w279 w288 w292 w307 w328 w368 w405 w442 w470 w482 w498 w518 w528 w539 w552 w558]
          tunnel: [w29 w41 w87 w93 w107 w113 w119 w124 w133 w141 w147 w156 w164 w172 w178 w192 w211 w219 w231 w239 w245 w251 w259 w267 w275 w283 w289 w302 w308 w319 w363 w400 w437 w472 w484 w489 w510 w524 w535 w549 w559] -> w23
          tunnel: w22 -> [w29 w44 w87 w92 w107 w113 w119 w123 w133 w141 w147 w156 w164 w172 w178 w192 w210 w218 w230 w239 w245 w251 w259 w267 w275 w283 w289 w302 w308 w331 w357 w394 w431 w472 w484 w495 w509 w523 w534 w548 w559]
          tunnel: [w28 w55 w85 w98 w105 w112 w118 w127 w132 w139 w146 w155 w162 w170 w177 w182 w207 w222 w227 w238 w244 w249 w257 w265 w273 w280 w288 w293 w307 w329 w369 w406 w443 w471 w483 w499 w519 w529 w540 w553 w558] -> w21
          tunnel: ["Timeout" w42 "Overwrite Value Change Event" "Voltage Color Scale Value Change Event" "Pixellate Value Change Event" "Archive Value Change Event" "Unarchive Value Change Event" "Zoom Tool Autoselection" "Image Data Range Sliding Ended" "Autosave Render Event Value Changed" "Save Render Value Change Event" "Copy Render Value Change Event" "Normal Save Path Value Change Event" "Autosave Path Value Change Event" "Inset Editor Opened" "Render Mouse Down Event" "Filter Render Mouse Down Event" "Help Value Change Event" "Lithography ABORT Called" "Refresh Value Change Event" "Done Value Change Event" "Lithography Value Change Event" "Inkscape file Value Change Event" "Background file Value Change Event" "Image Data Range Value Change Event" "Page Value Change Event" "Zoom to Fit Event" "Show-Hide Labels Event" "AFM Lithography Finished Event" w312 w350 w387 w425 "Tooled Objects Recieved from Tooler" "Parsed Data Recieved" "Multicolumn Listbox Value Change Event" "MCLB Click" ("t") "MCLB Drag Ended" ("t") _ "Multicolumn Listbox RCM Selection Event" _] -> w18
          event Timeout {
            # "Timeout Frame\n(this will only execute if the Event Structure timeout is >= 0)"
            n6 = event-data() -> ()  [unwired: 1 in, 1 out]
            n7 = call <vilib>:"Add State(s) to Queue__jki_lib_state_machine.vi"("State(s) in (\"\")"=w31) -> ("States Out"=w30:string)  [unwired: 14 in]
          }
          event "Tab Selectors": Value Change {
            # "Timeout Frame\n(this will only execute if the Event Structure timeout is >= 0)"
            n8 = event-data() -> ("NewVal"=w45:T1)  [unwired: 1 in]
            n9 = Format Into String(initial string="New tab selected: ", error in=w44, w45) -> (resulting string=w42:string, error out=w36:errorcluster)  [unwired: 1 in]
            n10 = case shown="\"Home\"" w45 {
              tunnel: [u32 6316128 ("Boolean Text.Text Colors:Text Color") u32 6316128 ("Boolean Text.Text Colors:Text Color") u32 6316128 ("Boolean Text.Text Colors:Text Color") u32 2829099 ("Boolean Text.Text Colors:Text Color")] -> w50
              tunnel: [u32 6316128 ("Boolean Text.Text Colors:Text Color") u32 2829099 ("Boolean Text.Text Colors:Text Color") u32 6316128 ("Boolean Text.Text Colors:Text Color") u32 6316128 ("Boolean Text.Text Colors:Text Color")] -> w48
              tunnel: [u32 6316128 ("Boolean Text.Text Colors:Text Color") u32 6316128 ("Boolean Text.Text Colors:Text Color") u32 2829099 ("Boolean Text.Text Colors:Text Color") u32 6316128 ("Boolean Text.Text Colors:Text Color")] -> w47
              tunnel: [u32 2829099 ("Boolean Text.Text Colors:Text Color") u32 6316128 ("Boolean Text.Text Colors:Text Color") u32 6316128 ("Boolean Text.Text Colors:Text Color") u32 6316128 ("Boolean Text.Text Colors:Text Color")] -> w49
              tunnel: [T3."Patterns and Writing" ("Settings") T3."AFM Settings" ("Settings") T3."Image Settings" ("Settings") T3."Program Settings" ("Settings")] -> w46
              tunnel: [_ _ TRUE _] -> w35
              tunnel: [_ TRUE _ _] -> w34
              tunnel: [TRUE _ _ _] -> w33
              tunnel: [_ _ _ TRUE] -> w32
              frame "Patterns" {
              }
              frame "Microscope" {
              }
              frame "Image" {
              }
              frame "Home" {
              }
            }
            n11 = local write "Settings"(w46) -> ()
            n12 = control-ref of="Home"() -> (w54:refnum<vi>)
            n13 = control-ref of="Patterns"() -> (w53:refnum<vi>)
            n14 = control-ref of="Microscope"() -> (w52:refnum<vi>)
            n15 = control-ref of="Image"() -> (w51:refnum<vi>)
            n16 = property class="Bool (strict)"(reference=w54, error in=w36, "BoolText.TextColor"=w50, "BoolText.FontBold"=w32) -> (error out=w40:errorcluster)  [unwired: 1 out]
            n17 = property class="Bool (strict)"(reference=w53, error in=w36, "BoolText.TextColor"=w49, "BoolText.FontBold"=w33) -> (error out=w39:errorcluster)  [unwired: 1 out]
            n18 = property class="Bool (strict)"(reference=w52, error in=w36, "BoolText.TextColor"=w48, "BoolText.FontBold"=w34) -> (error out=w38:errorcluster)  [unwired: 1 out]
            n19 = property class="Bool (strict)"(reference=w51, error in=w36, "BoolText.TextColor"=w47, "BoolText.FontBold"=w35) -> (error out=w37:errorcluster)  [unwired: 1 out]
            n20 = Merge Errors(w40, w39, w38, w37, w36) -> (w41:errorcluster)
            n21 = call <vilib>:"Add State(s) to Queue__jki_lib_state_machine.vi"("State(s) in (\"\")"=w57) -> ("States Out"=w56:string)  [unwired: 14 in]
          }
          event "Overwrite?": Value Change {
            # "Timeout Frame\n(this will only execute if the Event Structure timeout is >= 0)"
            n22 = event-data() -> ("NewVal"=w83:bool)  [unwired: 1 in, 5 out]
            n23 = Bundle By Name(cluster=w84, "UI.Overwrite"=w83) -> (w85:T25)
            n24 = call <vilib>:"Add State(s) to Queue__jki_lib_state_machine.vi"("State(s) in Front (\"\")"="Config: Write", "State(s) in (\"\")"=w89) -> ("States Out"=w88:string)  [unwired: 13 in]
          }
          event "Voltage Color Scale": Value Change {
            # "Timeout Frame\n(this will only execute if the Event Structure timeout is >= 0)"
            n25 = event-data() -> ("NewVal"=w91:dbl)  [unwired: 1 in, 5 out]
            n26 = Absolute Value(x=w91) -> (abs(x)=w90:dbl)
            n27 = Unbundle By Name(w96) -> ("big-maq"=w95:refnum<class "BigMAQ.lvclass">)
            n28 = call-dynamic "Write Voltage Scale.vi"("error in (no error)"=w92, "Voltage Scale"=w90, "BigMAQ in"=w95) -> ("error out"=w93:errorcluster, "BigMAQ out"=w94:refnum<class "BigMAQ.lvclass">)  [unwired: 7 in]
            n29 = Bundle By Name(cluster=w96, "big-maq"=w94) -> (w98:T25)
            n30 = call <vilib>:"Add State(s) to Queue__jki_lib_state_machine.vi"("State(s) in Front (\"\")"="Big MAQ: Generate Overlay\nBig MAQ: Update", "State(s) in (\"\")"=w101) -> ("States Out"=w100:string)  [unwired: 13 in]
          }
          event "Pixellate?": Value Change {
            # "Timeout Frame\n(this will only execute if the Event Structure timeout is >= 0)"
            n31 = event-data() -> ("NewVal"=w102:bool)  [unwired: 1 in, 5 out]
            n32 = local write "Slow Alert"(w102) -> ()
            n33 = Bundle By Name(cluster=w104, "UI.Pixellate?"=w102) -> (w105:T25)
            n34 = call <vilib>:"Add State(s) to Queue__jki_lib_state_machine.vi"("State(s) in Front (\"\")"="UI: Update Control >> Ready >> False\nBig MAQ: Generate Overlay\nBig MAQ: Update\nUI: Update Control >> Ready >> True", "State(s) in (\"\")"=w109) -> ("States Out"=w108:string)  [unwired: 13 in]
          }
          event "Archive": Value Change {
            # "Timeout Frame\n(this will only execute if the Event Structure timeout is >= 0)"
            n35 = event-data() -> ()  [unwired: 1 in, 6 out]
            n36 = call <vilib>:"Add State(s) to Queue__jki_lib_state_machine.vi"("State(s) in Front (\"\")"="Archivist: Location >> Archive\nArchivist: Archive", "State(s) in (\"\")"=w115) -> ("States Out"=w114:string)  [unwired: 13 in]
          }
          event "Unarchive": Value Change {
            # "Timeout Frame\n(this will only execute if the Event Structure timeout is >= 0)"
            n37 = event-data() -> ()  [unwired: 1 in, 6 out]
            n38 = call <vilib>:"Add State(s) to Queue__jki_lib_state_machine.vi"("State(s) in Front (\"\")"="UI: Update Control >> Ready >> False\nArchivist: Location >> Unarchive\nArchivist: Unarchive\nUI: Update Control >> Background Image\nUI: Update Control >> Inkscape\n//File: Background\nBig MAQ: Read Background\nAFM: Background Image\n//Big MAQ: Generate Overlay\nBig MAQ: Update\n//UI: Update Control >> Ready >> True\n//UI: Update Control >> Ready >> False\nParse: Send File\nConfig: Write\nBig MAQ: Save Background", "State(s) in (\"\")"=w121) -> ("States Out"=w120:string)  [unwired: 13 in]
          }
          event "Zoom Type", "Zoom to Fit": Mouse Down {
            w122 = u32 8 items=["Zoom Tool"=8, "Selection Tool"=0, "Pan Tool"=9, "Point Tool"=1, "Line Tool"=2, "Rectangle Tool"=3, "Rotated Rectangle Tool"=12, "Polyline Tool"=10, "Polygon Tool"=5, "Freehand Tool"=11, "Closed Freehand Tool"=6, "Ellipse Tool"=4, "Annulus Tool"=7] ("Current ROI Tool")
            # "Timeout Frame\n(this will only execute if the Event Structure timeout is >= 0)"
            n39 = event-data() -> ()  [unwired: 1 in, 8 out]
            n40 = control-ref of="Render"() -> (w125:refnum<vi>)
            n41 = property class="ImageControl"(reference=w125, error in=w123, "Current ROI Tool"=w122) -> (error out=w124:errorcluster)  [unwired: 1 out]
            n42 = call <vilib>:"Add State(s) to Queue__jki_lib_state_machine.vi"("State(s) in (\"\")"=w129) -> ("States Out"=w128:string)  [unwired: 14 in]
          }
          event "Image Data Range": Mouse Up {
            # "Timeout Frame\n(this will only execute if the Event Structure timeout is >= 0)"
            n43 = event-data() -> ()  [unwired: 1 in, 8 out]
            n44 = call <vilib>:"Add State(s) to Queue__jki_lib_state_machine.vi"("State(s) in Front (\"\")"="Big MAQ: Save Background" ("State(s) in Front (\"\")"), "State(s) in (\"\")"=w135) -> ("States Out"=w134:string)  [unwired: 13 in]
          }
          event "Autosave?": Value Change {
            # "Timeout Frame\n(this will only execute if the Event Structure timeout is >= 0)"
            n45 = event-data() -> ("NewVal"=w137:bool)  [unwired: 1 in, 5 out]
            n46 = Bundle By Name(cluster=w138, "UI.Autosave?"=w137) -> (w139:T25)
            n47 = call <vilib>:"Add State(s) to Queue__jki_lib_state_machine.vi"("State(s) in Front (\"\")"="Config: Write", "State(s) in (\"\")"=w143) -> ("States Out"=w142:string)  [unwired: 13 in]
          }
          event "Save Render": Value Change {
            # "Timeout Frame\n(this will only execute if the Event Structure timeout is >= 0)"
            n48 = event-data() -> ()  [unwired: 1 in, 6 out]
            n49 = call <vilib>:"Add State(s) to Queue__jki_lib_state_machine.vi"("State(s) in Front (\"\")"="Big MAQ: Save Render", "State(s) in (\"\")"=w149) -> ("States Out"=w148:string)  [unwired: 13 in]
          }
          event "CopyRender": Value Change {
            # "Timeout Frame\n(this will only execute if the Event Structure timeout is >= 0)"
            n50 = event-data() -> ("NewVal"=w150:bool)  [unwired: 1 in]
            n51 = Select(t="", s=w150, f="Big MAQ: Copy Render") -> (s? t:f=w151:string)
            n52 = call <vilib>:"Add State(s) to Queue__jki_lib_state_machine.vi"("State(s) in Front (\"\")"=w151, "State(s) in (\"\")"=w158) -> ("States Out"=w157:string)  [unwired: 13 in]
          }
          event "Normal Save Path": Value Change {
            # "Timeout Frame\n(this will only execute if the Event Structure timeout is >= 0)"
            n53 = event-data() -> ("NewVal"=w160:path)  [unwired: 1 in, 5 out]
            n54 = Bundle By Name(cluster=w161, "UI.Normal Save Path"=w160) -> (w162:T25)
            n55 = call <vilib>:"Add State(s) to Queue__jki_lib_state_machine.vi"("State(s) in Front (\"\")"="Config: Write", "State(s) in (\"\")"=w166) -> ("States Out"=w165:string)  [unwired: 13 in]
          }
          event "Autosave Path": Value Change {
            # "Timeout Frame\n(this will only execute if the Event Structure timeout is >= 0)"
            n56 = event-data() -> ("NewVal"=w168:path)  [unwired: 1 in, 5 out]
            n57 = Bundle By Name(cluster=w169, "UI.Autosave Path"=w168) -> (w170:T25)
            n58 = call <vilib>:"Add State(s) to Queue__jki_lib_state_machine.vi"("State(s) in Front (\"\")"="Config: Write", "State(s) in (\"\")"=w174) -> ("States Out"=w173:string)  [unwired: 13 in]
          }
          event "Inset Editor": Value Change {
            # "Timeout Frame\n(this will only execute if the Event Structure timeout is >= 0)"
            n59 = event-data() -> ()  [unwired: 1 in, 6 out]
            n60 = call <vilib>:"Add State(s) to Queue__jki_lib_state_machine.vi"("State(s) in Front (\"\")"="UI: Create Insert", "State(s) in (\"\")"=w180) -> ("States Out"=w179:string)  [unwired: 13 in]
          }
          event "Render": Mouse Down {
            w185 = u32 8 items=["Zoom Tool"=8, "Selection Tool"=0, "Pan Tool"=9, "Point Tool"=1, "Line Tool"=2, "Rectangle Tool"=3, "Rotated Rectangle Tool"=12, "Polyline Tool"=10, "Polygon Tool"=5, "Freehand Tool"=11, "Closed Freehand Tool"=6, "Ellipse Tool"=4, "Annulus Tool"=7] ("Current ROI Tool")
            # "Zoom factor implemented here will be nice."
            # "Timeout Frame\n(this will only execute if the Event Structure timeout is >= 0)"
            n61 = event-data() -> ("CtlRef"=w189:refnum<vi>)  [unwired: 1 in]
            n62 = Unbundle By Name(w181) -> ("Zoom History"=w188:cluster{"X":sgl, "Y":sgl}[])
            n63 = property class="ImageControl"(reference=w189) -> ("ZoomSingle"=w187:cluster{"X":sgl, "Y":sgl}, "Current ROI Tool"=w186:u32)  [unwired: 1 in, 2 out]
            n64 = Equal?(x=w186, y=w185) -> (x = y?=w184:bool)
            n65 = case shown="True" w184 {
              tunnel: w188 -> [w195 w200]
              tunnel: w187 -> [_ w199]
              tunnel: [w195 w196] -> w183
              frame False {
              }
              frame True {
                n66 = Build Array (concatenate)(w200, w199) -> (w198:cluster{"X":sgl, "Y":sgl}[])
                n67 = Sort 1D Array(array=w198) -> (sorted array=w197:cluster{"X":sgl, "Y":sgl}[])
                n68 = call "Remove Duplicates From 1D Array.vim"("array"=w197) -> ("array with duplicates removed"=w196:cluster{"X":sgl, "Y":sgl}[])  [unwired: 10 in]
              }
            }
            n69 = Bundle By Name(cluster=w181, "Zoom History"=w183) -> (w182:T25)
            n70 = call <vilib>:"Add State(s) to Queue__jki_lib_state_machine.vi"("State(s) in Front (\"\")"="UI: Update Zoom Factor", "State(s) in (\"\")"=w194) -> ("States Out"=w193:string)  [unwired: 13 in]
          }
          event "Render": Mouse Down? {
            # "Hold shift if we are zooming out"
            # "Discard when we manually set zoom"
            # "Zoom factor implemented here will be nice."
            # "Timeout Frame\n(this will only execute if the Event Structure timeout is >= 0)"
            n71 = event-data() -> ("Coords"=w205:T26)  [unwired: 1 in, 1 out]
            n72 = Unbundle By Name(w206) -> ("big-maq"=w213:refnum<class "BigMAQ.lvclass">, "Zoom History"=w214:cluster{"X":sgl, "Y":sgl}[])
            n73 = local read "Zoom Type"() -> (w212:enum32{"Zoom In", "Zoom Out"})
            n74 = call "Handle Zoom Event.vi"("Point32"=w205, "error in"=w210, "Zoom History"=w214, "Zoom Type"=w212, "BigMAQ in"=w213) -> ("error out"=w211:errorcluster, "Discard?"=w203:bool, "Zoom Out?"=w209:bool, "BigMAQ out"=w208:refnum<class "BigMAQ.lvclass">)  [unwired: 3 in]
            n75 = Bundle By Name(cluster=w206, "big-maq"=w208) -> (w207:T25)
            n76 = Select(t="UI: Update Zoom Factor", s=w203, f="") -> (s? t:f=w201:string)
            n77 = event-data("PlatMods.Shift"=w209, "Discard?"=w203) -> ()  [unwired: 3 in, 1 out]
            n78 = call <vilib>:"Add State(s) to Queue__jki_lib_state_machine.vi"("State(s) in Front (\"\")"=w201, "State(s) in (\"\")"=w217) -> ("States Out"=w216:string)  [unwired: 13 in]
          }
          event "Help": Value Change {
            # "Timeout Frame\n(this will only execute if the Event Structure timeout is >= 0)"
            n79 = event-data() -> ()  [unwired: 1 in, 6 out]
            n80 = call-poly <vilib>:"Open URL in Default Browser.vi"("error in (no error)"=w218, "URL"="https://github.com/levylabpitt/AFM-Lithography") -> ("error out"=w219:errorcluster)  [unwired: 4 in, 1 out]
            n81 = call <vilib>:"Add State(s) to Queue__jki_lib_state_machine.vi"("State(s) in (\"\")"=w224) -> ("States Out"=w223:string)  [unwired: 14 in]
          }
          event "Abort": Value Change {
            # "Abort: Value Change\n(this will only execute if the Event Structure timeout is >= 0)"
            n82 = event-data() -> ()  [unwired: 1 in, 6 out]
            n83 = Unbundle By Name(w226) -> ("afm_mngr"=w232:refnum<class "AFM_Driver_Manager.lvclass">)
            n84 = call "AFM_Driver_Manager.Abort.vi"("AFM_Driver_Manager in"=w232) -> ("error out"=w229:errorcluster, "AFM_Driver_Manager out"=w228:refnum<class "AFM_Driver_Manager.lvclass">)  [unwired: 9 in]
            n85 = Bundle By Name(cluster=w226, "afm_mngr"=w228) -> (w227:T25)
            n86 = Merge Errors(w229, w230) -> (w231:errorcluster)
            n87 = call <vilib>:"Add State(s) to Queue__jki_lib_state_machine.vi"("State(s) in Front (\"\")"="UI: Enable Run >> Enabled" ("State(s) in Front (\"\")"), "State(s) in (\"\")"=w235) -> ("States Out"=w234:string)  [unwired: 13 in]
          }
          event "Refresh Button": Value Change {
            # "This should just call what would be called when we have a new ibw and new svg file"
            # "Refresh: Value Change\n(this will only execute if the Event Structure timeout is >= 0)"
            n88 = event-data() -> ()  [unwired: 1 in, 6 out]
            n89 = call <vilib>:"Add State(s) to Queue__jki_lib_state_machine.vi"("State(s) in Front (\"\")"="UI: Update Control >> Ready >> False\nFile: Background\nFile: Inkscape\nBig MAQ: Read Background\nParse: Send File\nAFM: Background Image", "State(s) in (\"\")"=w241) -> ("States Out"=w240:string)  [unwired: 13 in]
          }
          event "Done": Value Change {
            # "Abort: Value Change\n(this will only execute if the Event Structure timeout is >= 0)"
            n90 = event-data() -> ()  [unwired: 1 in, 6 out]
            n91 = call <vilib>:"Add State(s) to Queue__jki_lib_state_machine.vi"("State(s) in Front (\"\")"="Macro: Exit" ("State(s) in Front (\"\")"), "State(s) in (\"\")"=w247) -> ("States Out"=w246:string)  [unwired: 13 in]
          }
          event "Run": Value Change {
            # "Run: Value Change\n(this will only execute if the Event Structure timeout is >= 0)"
            n92 = event-data() -> ()  [unwired: 1 in, 6 out]
            n93 = call <vilib>:"Add State(s) to Queue__jki_lib_state_machine.vi"("State(s) in Front (\"\")"="UI: Enable Run >> Disabled\nAFM: Run Lithography\nBig MAQ: Autosave Render", "State(s) in (\"\")"=w253) -> ("States Out"=w252:string)  [unwired: 13 in]
          }
          event "Inkscape File (.svg)": Value Change {
            # "Inkscape: Value Change\n(this will only execute if the Event Structure timeout is >= 0)"
            n94 = event-data() -> ("NewVal"=w255:path)  [unwired: 1 in, 5 out]
            n95 = Bundle By Name(cluster=w256, "UI.Inkscape File (.svg)"=w255) -> (w257:T25)
            n96 = call <vilib>:"Add State(s) to Queue__jki_lib_state_machine.vi"("State(s) in Front (\"\")"="UI: Update Control >> Ready >> False\nParse: Send File\nConfig: Write\nBig MAQ: Save Background", "State(s) in (\"\")"=w261) -> ("States Out"=w260:string)  [unwired: 13 in]
          }
          event "Background Image": Value Change {
            # "Background: Value Change\n(this will only execute if the Event Structure timeout is >= 0)"
            n97 = event-data() -> ("NewVal"=w263:path)  [unwired: 1 in, 5 out]
            n98 = Bundle By Name(cluster=w264, "UI.Background Image"=w263) -> (w265:T25)
            n99 = call <vilib>:"Add State(s) to Queue__jki_lib_state_machine.vi"("State(s) in Front (\"\")"="UI: Update Control >> Ready >> False\nFile: Background\nBig MAQ: Read Background\nBig MAQ: Coerce Size\nAFM: Background Image\nBig MAQ: Generate Overlay\nBig MAQ: Update\nUI: Update Control >> Ready >> True" ("State(s) in Front (\"\")"), "State(s) in (\"\")"=w269) -> ("States Out"=w268:string)  [unwired: 13 in]
          }
          event "Image Data Range": Value Change {
            # "Image Data Range: Value Change\n(Only the most recent event in the queue is here..."
            n100 = event-data() -> ("NewVal"=w271:cluster{sgl, sgl})  [unwired: 1 in, 5 out]
            n101 = Bundle By Name(cluster=w272, "UI.Image Data Range"=w271) -> (w273:T25)
            n102 = call <vilib>:"Add State(s) to Queue__jki_lib_state_machine.vi"("State(s) in Front (\"\")"="Big MAQ: Change Data Range\nBig MAQ: Update", "State(s) in (\"\")"=w277) -> ("States Out"=w276:string)  [unwired: 13 in]
          }
          event "Data Channel": Value Change {
            # "Page: Value Change\n(this will only execute if the Event Structure timeout is >= 0)"
            n103 = event-data() -> ("NewVal"=w278:u32)  [unwired: 1 in, 5 out]
            n104 = Bundle By Name(cluster=w279, "UI.Page"=w278) -> (w280:T25)
            n105 = call <vilib>:"Add State(s) to Queue__jki_lib_state_machine.vi"("State(s) in Front (\"\")"="Big MAQ: Select Page\nBig MAQ: Change Data Range\nBig MAQ: Update", "State(s) in (\"\")"=w285) -> ("States Out"=w284:string)  [unwired: 13 in]
          }
          event "Zoom to Fit": Value Change {
            # "Timeout Frame\n(this will only execute if the Event Structure timeout is >= 0)"
            n106 = event-data() -> ()  [unwired: 1 in, 6 out]
            n107 = call <vilib>:"Add State(s) to Queue__jki_lib_state_machine.vi"("State(s) in Front (\"\")"="Big MAQ: Zoom Fit\nUI: Update Zoom Factor", "State(s) in (\"\")"=w291) -> ("States Out"=w290:string)  [unwired: 13 in]
          }
          event "Hide Labels?": Value Change {
            # "Timeout Frame\n(this will only execute if the Event Structure timeout is >= 0)"
            n108 = event-data() -> ("NewVal"=w294:bool)  [unwired: 1 in, 5 out]
            n109 = Bundle By Name(cluster=w292, "UI.Hide Labels"=w294) -> (w293:T25)
            n110 = Select(t="show", s=w294, f="hide") -> (s? t:f=w300:string)
            n111 = call <vilib>:"Build State String with Arguments__JKI_lib_State_Machine.vi"("Arguments (\"\")"=w300, "State"="Big MAQ: Labels") -> ("State with Arguments"=w298:string)  [unwired: 4 in]
            n112 = call <vilib>:"Add State(s) to Queue__jki_lib_state_machine.vi"("State(s) in Front (\"\")"=w298, "State(s) in (\"\")"=w304, "State(s) at Back (\"\")"="Big MAQ: Update" ("State(s) at Back (\"\")")) -> ("States Out"=w303:string)  [unwired: 12 in]
          }
          event User Event {
            # "Timeout Frame\n(this will only execute if the Event Structure timeout is >= 0)"
            n113 = event-data() -> ()  [unwired: 1 in, 5 out]
            n114 = call <vilib>:"Add State(s) to Queue__jki_lib_state_machine.vi"("State(s) in Front (\"\")"="UI: Enable Run >> Enabled\nAFM: Lithography Finished", "State(s) in (\"\")"=w310) -> ("States Out"=w309:string)  [unwired: 13 in]
          }
          event User Event {
            # "Timeout Frame\n(this will only execute if the Event Structure timeout is >= 0)"
            n115 = event-data() -> ("Read?"=w318:refnum<notifier>, "PathsUpdated"=w332:T18)  [unwired: 1 in]
            n116 = call "CheckIfEventRead.vi"("Read?"=w318) -> ("Read"=w311:bool)  [unwired: 9 in, 1 out]
            n117 = Unbundle By Name(w328) -> ("selector"=w327:refnum<class "Selector.lvclass">)
            n118 = for {
              tunnel: w332 -> [w340] mode=indexing
              tunnel: [w347] -> w324 mode=indexing
              tunnel: [w338] -> w325 mode=indexing
              shift-right: [w343] -> w320
              shift-left: w331 -> [w339]
              tunnel: [w346] -> w323 mode=indexing
              tunnel: [w344] -> w330 mode=indexing
              n119 = call-dynamic "Read GUID.vi"("error in (no error)"=w339, "ObjectSettings in"=w340) -> ("error out"=w336:errorcluster, "GUID"=w337:string, "ObjectSettings out"=w341:refnum<class "Path Settings.lvclass">)  [unwired: 7 in]
              n120 = call "Query Registry.vi"("error in"=w336, "Name In"=w337) -> ("error out"=w335:errorcluster, "Alias"=w338:string)  [unwired: 6 in, 2 out]
              n121 = call-dynamic "Read Group.vi"("error in (no error)"=w335, "ObjectSettings in"=w341) -> ("error out"=w342:errorcluster, "Group"=w346:string, "ObjectSettings out"=w345:refnum<class "Path Settings.lvclass">)  [unwired: 7 in]
              n122 = call "Read Enabled.vi"("error in (no error)"=w342, "ObjectSettings in"=w345) -> ("error out"=w343:errorcluster, "Enabled"=w347:bool, "ObjectSettings out"=w344:refnum<class "Path Settings.lvclass">)  [unwired: 7 in]
            }
            n123 = Select(t="", s=w311, f="Macro: Objects Updated" ("State(s) in Front (\"\")")) -> (s? t:f=w316:string)
            n124 = Bundle(cluster=T4 {"Groups"=[], "Enable Items"=[]} ("Settings"), "Groups"=w323, "Enable Items"=w324) -> (w322:T4)
            n125 = call "UI--Settings by Name.vi"("error in"=w320, "Settings"=w322, "Names"=w325, "Selector in"=w327) -> ("error out"=w319:errorcluster, "Selector out"=w326:refnum<class "Selector.lvclass">)  [unwired: 6 in]
            n126 = Bundle By Name(cluster=w328, "selector"=w326, "Obj Settings.Paths"=w330) -> (w329:T25)
            n127 = Select(t="Paths Updated: Ignored", s=w311, f="Paths Updated") -> (s? t:f=w312:string)
            n128 = call <vilib>:"Add State(s) to Queue__jki_lib_state_machine.vi"("State(s) in Front (\"\")"=w316, "State(s) in (\"\")"=w334) -> ("States Out"=w333:string)  [unwired: 13 in]
          }
          event User Event {
            # "Timeout Frame\n(this will only execute if the Event Structure timeout is >= 0)"
            n129 = event-data() -> ("Read?"=w354:refnum<notifier>, "RectanglesUpdated"=w358:T19)  [unwired: 1 in]
            n130 = call "CheckIfEventRead.vi"("Read?"=w354) -> ("Read"=w348:bool)  [unwired: 9 in, 1 out]
            n131 = Unbundle By Name(w368) -> ("selector"=w367:refnum<class "Selector.lvclass">)
            n132 = for {
              tunnel: w358 -> [w377] mode=indexing
              tunnel: [w384] -> w360 mode=indexing
              tunnel: [w375] -> w359 mode=indexing
              shift-right: [w380] -> w356
              shift-left: w357 -> [w376]
              tunnel: [w383] -> w361 mode=indexing
              tunnel: [w381] -> w355 mode=indexing
              n133 = call-dynamic "Read GUID.vi"("error in (no error)"=w376, "ObjectSettings in"=w377) -> ("error out"=w373:errorcluster, "GUID"=w374:string, "ObjectSettings out"=w378:refnum<class "Rectangle Settings.lvclass">)  [unwired: 7 in]
              n134 = call "Query Registry.vi"("error in"=w373, "Name In"=w374) -> ("error out"=w372:errorcluster, "Alias"=w375:string)  [unwired: 6 in, 2 out]
              n135 = call-dynamic "Read Group.vi"("error in (no error)"=w372, "ObjectSettings in"=w378) -> ("error out"=w379:errorcluster, "Group"=w383:string, "ObjectSettings out"=w382:refnum<class "Rectangle Settings.lvclass">)  [unwired: 7 in]
              n136 = call "Read Enabled.vi"("error in (no error)"=w379, "ObjectSettings in"=w382) -> ("error out"=w380:errorcluster, "Enabled"=w384:bool, "ObjectSettings out"=w381:refnum<class "Rectangle Settings.lvclass">)  [unwired: 7 in]
            }
            n137 = Bundle(cluster=T4 {"Groups"=[], "Enable Items"=[]} ("Settings"), "Groups"=w361, "Enable Items"=w360) -> (w365:T4)
            n138 = call "UI--Settings by Name.vi"("error in"=w356, "Settings"=w365, "Names"=w359, "Selector in"=w367) -> ("error out"=w363:errorcluster, "Selector out"=w366:refnum<class "Selector.lvclass">)  [unwired: 6 in]
            n139 = Select(t="", s=w348, f="Macro: Objects Updated" ("State(s) in Front (\"\")")) -> (s? t:f=w351:string)
            n140 = Bundle By Name(cluster=w368, "selector"=w366, "Obj Settings.Rectangles"=w355) -> (w369:T25)
            n141 = Select(t="Rectangles Updated: Ignored", s=w348, f="Rectangles Updated") -> (s? t:f=w350:string)
            n142 = call <vilib>:"Add State(s) to Queue__jki_lib_state_machine.vi"("State(s) in Front (\"\")"=w351, "State(s) in (\"\")"=w371) -> ("States Out"=w370:string)  [unwired: 13 in]
          }
          event User Event {
            # "Timeout Frame\n(this will only execute if the Event Structure timeout is >= 0)"
            n143 = event-data() -> ("Read?"=w391:refnum<notifier>, "FunnelsUpdated"=w395:T20)  [unwired: 1 in]
            n144 = call "CheckIfEventRead.vi"("Read?"=w391) -> ("Read"=w385:bool)  [unwired: 9 in, 1 out]
            n145 = Unbundle By Name(w405) -> ("selector"=w404:refnum<class "Selector.lvclass">)
            n146 = for {
              tunnel: w395 -> [w414] mode=indexing
              tunnel: [w421] -> w397 mode=indexing
              tunnel: [w412] -> w396 mode=indexing
              shift-right: [w417] -> w392
              shift-left: w394 -> [w413]
              tunnel: [w420] -> w398 mode=indexing
              tunnel: [w418] -> w393 mode=indexing
              n147 = call-dynamic "Read GUID.vi"("error in (no error)"=w413, "ObjectSettings in"=w414) -> ("error out"=w410:errorcluster, "GUID"=w411:string, "ObjectSettings out"=w415:refnum<class "Funnel Settings.lvclass">)  [unwired: 7 in]
              n148 = call "Query Registry.vi"("error in"=w410, "Name In"=w411) -> ("error out"=w409:errorcluster, "Alias"=w412:string)  [unwired: 6 in, 2 out]
              n149 = call-dynamic "Read Group.vi"("error in (no error)"=w409, "ObjectSettings in"=w415) -> ("error out"=w416:errorcluster, "Group"=w420:string, "ObjectSettings out"=w419:refnum<class "Funnel Settings.lvclass">)  [unwired: 7 in]
              n150 = call "Read Enabled.vi"("error in (no error)"=w416, "ObjectSettings in"=w419) -> ("error out"=w417:errorcluster, "Enabled"=w421:bool, "ObjectSettings out"=w418:refnum<class "Funnel Settings.lvclass">)  [unwired: 7 in]
            }
            n151 = Bundle(cluster=T4 {"Groups"=[], "Enable Items"=[]} ("Settings"), "Groups"=w398, "Enable Items"=w397) -> (w402:T4)
            n152 = Select(t="", s=w385, f="Macro: Objects Updated" ("State(s) in Front (\"\")")) -> (s? t:f=w389:string)
            n153 = call "UI--Settings by Name.vi"("error in"=w392, "Settings"=w402, "Names"=w396, "Selector in"=w404) -> ("error out"=w400:errorcluster, "Selector out"=w403:refnum<class "Selector.lvclass">)  [unwired: 6 in]
            n154 = Bundle By Name(cluster=w405, "selector"=w403, "Obj Settings.Funnels"=w393) -> (w406:T25)
            n155 = Select(t="Funnels Updated: Ignored", s=w385, f="Funnels Updated") -> (s? t:f=w387:string)
            n156 = call <vilib>:"Add State(s) to Queue__jki_lib_state_machine.vi"("State(s) in Front (\"\")"=w389, "State(s) in (\"\")"=w408) -> ("States Out"=w407:string)  [unwired: 13 in]
          }
          event User Event {
            # "Timeout Frame\n(this will only execute if the Event Structure timeout is >= 0)"
            n157 = event-data() -> ("Read?"=w429:refnum<notifier>, "DotsUpdated"=w430:T21)  [unwired: 1 in]
            n158 = call "CheckIfEventRead.vi"("Read?"=w429) -> ("Read"=w422:bool)  [unwired: 9 in, 1 out]
            n159 = Unbundle By Name(w442) -> ("selector"=w441:refnum<class "Selector.lvclass">)
            n160 = for {
              tunnel: [w458] -> w434 mode=indexing
              tunnel: [w450] -> w436 mode=indexing
              shift-right: [w454] -> w432
              shift-left: w431 -> [w451]
              tunnel: [w457] -> w435 mode=indexing
              tunnel: [w455] -> w433 mode=indexing
              tunnel: w430 -> [w446] mode=indexing
              n161 = call-dynamic "Read GUID.vi"("error in (no error)"=w451, "ObjectSettings in"=w446) -> ("error out"=w448:errorcluster, "GUID"=w449:string, "ObjectSettings out"=w452:refnum<class "Dot Settings.lvclass">)  [unwired: 7 in]
              n162 = call "Query Registry.vi"("error in"=w448, "Name In"=w449) -> ("error out"=w447:errorcluster, "Alias"=w450:string)  [unwired: 6 in, 2 out]
              n163 = call-dynamic "Read Group.vi"("error in (no error)"=w447, "ObjectSettings in"=w452) -> ("error out"=w453:errorcluster, "Group"=w457:string, "ObjectSettings out"=w456:refnum<class "Dot Settings.lvclass">)  [unwired: 7 in]
              n164 = call "Read Enabled.vi"("error in (no error)"=w453, "ObjectSettings in"=w456) -> ("error out"=w454:errorcluster, "Enabled"=w458:bool, "ObjectSettings out"=w455:refnum<class "Dot Settings.lvclass">)  [unwired: 7 in]
            }
            n165 = Select(t="", s=w422, f="Macro: Objects Updated" ("State(s) in Front (\"\")")) -> (s? t:f=w427:string)
            n166 = Bundle(cluster=T4 {"Groups"=[], "Enable Items"=[]} ("Settings"), "Groups"=w435, "Enable Items"=w434) -> (w439:T4)
            n167 = call "UI--Settings by Name.vi"("error in"=w432, "Settings"=w439, "Names"=w436, "Selector in"=w441) -> ("error out"=w437:errorcluster, "Selector out"=w440:refnum<class "Selector.lvclass">)  [unwired: 6 in]
            n168 = Bundle By Name(cluster=w442, "selector"=w440, "Obj Settings.Dots"=w433) -> (w443:T25)
            n169 = Select(t="Dots Updated: Ignored", s=w422, f="Dots Updated") -> (s? t:f=w425:string)
            n170 = call <vilib>:"Add State(s) to Queue__jki_lib_state_machine.vi"("State(s) in Front (\"\")"=w427, "State(s) in (\"\")"=w445) -> ("States Out"=w444:string)  [unwired: 13 in]
          }
          event User Event {
            n171 = event-data() -> ("Paths"=w464:refnum<class "Tool Path.lvclass">[], "Funnels"=w463:refnum<class "Tool Funnel.lvclass">[], "Rectangles"=w462:refnum<class "Tool Rectangle.lvclass">[], "Dots"=w461:refnum<class "Tool Dots.lvclass">[])  [unwired: 1 in, 4 out]
            n172 = Unbundle By Name(w470) -> ("tooler"=w468:refnum<class "Tool Data.lvclass">)
            n173 = property class="Tool Data.lvclass"(reference=w468) -> (reference out=w469:refnum<class "Tool Data.lvclass">, "Accessors:Tooled"=w466:T27)  [unwired: 1 in, 1 out]
            n174 = Bundle By Name(cluster=w466, "Paths"=w464, "Funnels"=w463, "Rectangles"=w462, "Dots"=w461) -> (w465:T27)
            n175 = property class="Tool Data.lvclass"(reference=w469, "Accessors:Tooled"=w465) -> (reference out=w467:refnum<class "Tool Data.lvclass">)  [unwired: 1 in, 1 out]
            n176 = Bundle By Name(cluster=w470, "tooler"=w467) -> (w471:T25)
            n177 = call <vilib>:"Add State(s) to Queue__jki_lib_state_machine.vi"("State(s) in Front (\"\")"="UI: Update Control >> Ready >> False\nTool: Generate Litho Data\nSelect: Order Litho\nBig MAQ: Coerce Size\nBig MAQ: Generate Overlay\nBig MAQ: Update\nAFM: Lithography Data\nUI: Update Control >> Ready >> True" ("State(s) in Front (\"\")"), "State(s) in (\"\")"=w474) -> ("States Out"=w473:string)  [unwired: 13 in]
          }
          event User Event {
            # "Timeout Frame\n(this will only execute if the Event Structure timeout is >= 0)"
            n178 = event-data() -> ("Paths"=w478:refnum<class "Path.lvclass">[], "Rectangles"=w479:refnum<class "Rectangle.lvclass">[], "Background"=w480:refnum<class "SVGImage.lvclass">, "Dots"=w481:refnum<class "Dot.lvclass">[], "Other Images"=w475:refnum<class "SVGImage.lvclass">[])  [unwired: 1 in]
            n179 = Bundle By Name(cluster=w482, "Parsed Obj.Paths"=w478, "Parsed Obj.Rectangles"=w479, "Parsed Obj.Background"=w480, "Parsed Obj.Dots"=w481, "Parsed Obj.Other Images"=w475) -> (w483:T25)
            n180 = call <vilib>:"Add State(s) to Queue__jki_lib_state_machine.vi"("State(s) in Front (\"\")"="Tool: Sort Paths\nTool: Get IDs\nIdentity: Populate\nSelect: New Name Set\nSelect: Update\nSettings: Refresh\nSelect: Change By Name >> First", "State(s) in (\"\")"=w486) -> ("States Out"=w485:string)  [unwired: 13 in]
          }
          event "MCLB": Value Change {
            n181 = event-data() -> ()  [unwired: 1 in, 6 out]
            n182 = Unbundle By Name(w498) -> ("selector"=w497:refnum<class "Selector.lvclass">)
            n183 = call "Event--Value Change.vi"("error in"=w495, "Selector in"=w497) -> ("error out"=w490:errorcluster, "Name"=w491:string, "Selector out"=w496:refnum<class "Selector.lvclass">)  [unwired: 7 in]
            n184 = Bundle By Name(cluster=w498, "selector"=w496) -> (w499:T25)
            n185 = Search and Replace String(replace all?=TRUE ("replace all? (F)"), input string="Select: Reorder\nSettings: Set Active >> <state>\nSubpanel: Insert >> <state>" ("State(s) in Front (\"\")"), search string="<state>", replace string=w491, error in=w490) -> (result string=w488:string, error out=w489:errorcluster)  [unwired: 3 in, 2 out]
            n186 = call <vilib>:"Add State(s) to Queue__jki_lib_state_machine.vi"("State(s) in Front (\"\")"=w488, "State(s) in (\"\")"=w501) -> ("States Out"=w500:string)  [unwired: 13 in]
          }
          event "MCLB": Mouse Down? {
            n187 = event-data() -> ("Coords"=w514:T26, "Button"=w513:u16, "PlatMods"=w512:T28)  [unwired: 1 in]
            n188 = Unbundle By Name(w518) -> ("selector"=w517:refnum<class "Selector.lvclass">)
            n189 = Bundle By Name(cluster=T6 {"Point"={"Left"=0, "Top"=0}, "Button"=0, "PlatMods"={"Shift"=FALSE, "Ctrl"=FALSE, "Alt"=FALSE, "Cmd"=FALSE, "Opt"=FALSE}} ("Event Data"), "Point"=w514, "Button"=w513, "PlatMods"=w512) -> (w511:T6)
            n190 = call "Event--Mouse Down.vi"("error in"=w509, "Event Data"=w511, "Selector in"=w517) -> ("error out"=w510:errorcluster, "Enable Change"=w507:bool, "Name"=w505:string, "Selector out"=w516:refnum<class "Selector.lvclass">)  [unwired: 5 in]
            n191 = call <vilib>:"Build State String with Arguments__JKI_lib_State_Machine.vi"("Arguments (\"\")"=w505, "State"="Settings: Change Enable") -> ("State with Arguments"=w506:string)  [unwired: 4 in]
            n192 = Select(t=w506, s=w507, f="" ("State(s) in Front (\"\")")) -> (s? t:f=w503:string)
            n193 = Bundle By Name(cluster=w518, "selector"=w516) -> (w519:T25)
            n194 = event-data("Discard?"=w507) -> ()  [unwired: 1 in, 1 out]
            n195 = call <vilib>:"Add State(s) to Queue__jki_lib_state_machine.vi"("State(s) in Front (\"\")"=w503, "State(s) in (\"\")"=w521) -> ("States Out"=w520:string)  [unwired: 13 in]
          }
          event "MCLB": Drag Ended {
            n196 = event-data() -> ()  [unwired: 1 in, 5 out]
            n197 = Unbundle By Name(w528) -> ("selector"=w526:refnum<class "Selector.lvclass">)
            n198 = call "Event--Drag Ended.vi"("error in"=w523, "Selector in"=w526) -> ("error out"=w524:errorcluster, "Selector out"=w525:refnum<class "Selector.lvclass">)  [unwired: 8 in]
            n199 = Bundle By Name(cluster=w528, "selector"=w525) -> (w529:T25)
            n200 = call <vilib>:"Add State(s) to Queue__jki_lib_state_machine.vi"("State(s) in Front (\"\")"="Select: Reorder\nSelect: Order Litho\nBig MAQ: Generate Overlay\nBig MAQ: Update" ("State(s) in Front (\"\")"), "State(s) in (\"\")"=w531) -> ("States Out"=w530:string)  [unwired: 13 in]
          }
          event "MCLB": Shortcut Menu Activation? {
            n201 = event-data() -> ("MenuRef"=w533:refnum<k9>, "Coords"=w532:T26)  [unwired: 1 in, 5 out]
            n202 = Unbundle By Name(w539) -> ("selector"=w537:refnum<class "Selector.lvclass">)
            n203 = call "Event--Shortcut Menu Activation.vi"("error in"=w534, "Coords"=w532, "MenuRef"=w533, "Selector in"=w537) -> ("error out"=w535:errorcluster, "Selector out"=w536:refnum<class "Selector.lvclass">)  [unwired: 6 in]
            n204 = Bundle By Name(cluster=w539, "selector"=w536) -> (w540:T25)
            n205 = event-data() -> ()  [unwired: 2 in, 1 out]
            n206 = call <vilib>:"Add State(s) to Queue__jki_lib_state_machine.vi"("State(s) in Front (\"\")"="" ("State(s) in Front (\"\")"), "State(s) in (\"\")"=w542) -> ("States Out"=w541:string)  [unwired: 13 in]
          }
          event "MCLB": Shortcut Menu Selection (User) {
            n207 = event-data() -> ("ItemPath"=w547:string)  [unwired: 1 in]
            n208 = Unbundle By Name(w552) -> ("selector"=w551:refnum<class "Selector.lvclass">)
            n209 = call "Event--Shortcut Menu Selection.vi"("error in"=w548, "ItemPath"=w547, "Selector in"=w551) -> ("error out"=w549:errorcluster, "Selection"=w546:string, "Selector out"=w550:refnum<class "Selector.lvclass">)  [unwired: 6 in]
            n210 = call <vilib>:"Build State String with Arguments__JKI_lib_State_Machine.vi"("Arguments (\"\")"=w546, "State"="Select: Group" ("State(s) in Front (\"\")")) -> ("State with Arguments"=w544:string)  [unwired: 4 in]
            n211 = Bundle By Name(cluster=w552, "selector"=w550) -> (w553:T25)
            n212 = call <vilib>:"Add State(s) to Queue__jki_lib_state_machine.vi"("State(s) in Front (\"\")"=w544, "State(s) in (\"\")"=w555) -> ("States Out"=w554:string)  [unwired: 13 in]
          }
          event Panel Close? {
            # "Discard the event because we'll close the front panel ourselves in Macro: Exit"
            # "Close Panel button (pressed) Event\n(this executes Macro: Exit to terminate the VI)"
            n213 = event-data() -> ()  [unwired: 1 in, 1 out]
            n214 = disable-structure shown="TARGET_TYPE==RT" {
              disable-tunnel: [w562 "Macro: Exit"] -> w556
              frame condition #0 {
                n215 = Two Button Dialog(message="Do you really want to exit the lithography program?", 1:"Cancel" ("F button name (\"Cancel\")"), 2:"Close" ("T button name (\"OK\")")) -> (T button?=w564:bool)
                n216 = Select(t="Macro: Exit", s=w564, f="") -> (s? t:f=w562:string)
              }
              frame condition #1 (active) {
              }
            }
            n217 = event-data("Discard?"=TRUE) -> ()  [unwired: 1 in, 1 out]
            n218 = call <vilib>:"Add State(s) to Queue__jki_lib_state_machine.vi"("State(s) in Front (\"\")"=w556, "State(s) in (\"\")"=w561) -> ("States Out"=w560:string)  [unwired: 13 in]
          }
        }
      }
      frame "---------- Core ----------" {
        # "Do not put any code in this frame.\n(it is a separator no-op)"
        n219 = call <vilib>:"Add State(s) to Queue__jki_lib_state_machine.vi"("State(s) in (\"\")"=w574) -> ("States Out"=w573:string)  [unwired: 14 in]
      }
      frame Default {
        w586 = 42 items=["No error", "Argument error", "Memory is full", "Out of zone", "End of file", "File already open", "Generic file I/O error", "File not found", "File permission error", "Disk is full", "Duplicate path", "Too many files open", "System feature not enabled", "Resource file not found", "Cannot add resource", "Resource not found", "Image not found", "Image memory error", "Pen does not exist", "Config type invalid", "Config token not found", "Config parse error", "Config memory error", "Bad external code format", "Bad external code offset", "External code not present", "Null window", "Destroy window error", "Null menu", "Print aborted", "Bad print record", "Print driver error", "Windows error during printing", "Memory error during printing", "Print dialog error", "Generic print error", "Invalid device refnum", "Device not found", "Device parameter error", "Device unit error", "Cannot open device", "Device call aborted", "Generic error", "Cancelled by user", "Object ID too low", "Object ID too high", "Object not in heap", "Unknown heap", "Unknown object (invalid DefProc)", "Unknown object (DefProc not in table)", "Message out of range", "Invalid (null) method", "Unknown message", "Manager call not supported", "Bad address", "Network operation in progress", "Network operation timed out", "Connection is busy", "Network attribute not supported", "Network error", "Address in use", "System out of memory", "Connection aborted", "Connection refused", "Not connected", "Already connected", "Connection closed", "Initialization error (interapplication manager)", "Bad occurrence", "Wait on unbound occurrence handler", "Occurrence queue overflow", "Datalog type conflict", "Unused", "Unrecognized type (interapplication manager)", "Memory corrupt", "Failed to make temporary DLL", "Old CIN version", "Drag socket not found", "Failed to load drop-object", "Failed to register OLE object", "Failed to release OLE object", "Format specifier type mismatch", "Unknown format specifier", "Too few format specifiers", "Too many format specifiers", "Scan failed", "Newer CIN version", "Error converting to variant", "Runtime menu error", "Password tampered", "Variant attribute not found", "Incompatible variant data type", "Event data is not available", "Event Store is not present", "Occurrence is not found", "Event Queue is not created", "Event info is not available", "Refnum passed is NULL", "Error retrieving Class GUID", "Error retrieving CoClass GUID", "Error retrieving TypeLib GUID.", "Bad built application magic bytes.", "Specific driver is different from the specific driver associated with the Logical Name.", "There is no session opened to the class driver.", "Max Error", "MAX - Error with config objects", "MAX - Error loading configuration", "MAX - Group not supported"]
        # "State Syntax:\nStateCategory: State >> Argument\nLine Terminator: Line feed\nExample:\nUI: Help >> About\n\nWhere \"UI\" is the state category\nWhere \"Help\" is the state\nWhere \"About\" is the argument\nOther Examples:\nApp Data: Initialize\nUI: Initialize\nHelp >> About\n\nCommenting:\nTo add a comment use \"//\" or \"#\" and all text to the right will be ignored\nCommenting Example:\nUI: Initialize // This initializes the UI\n# This whole line is a comment\n// Another comment line"
        # "Current State"
        # "Do not delete, rename, or modify this frame.\n(this is used to capture unhandled states and typos)"
        # "Handle mistyped state name (developer tool)"
        n220 = Format Into String(format string="Software Exception: Unhandled State \"%s\"." ("message"), error in=w582, w577) -> (resulting string=w585:string, error out=w584:errorcluster)  [unwired: 1 in]
        n221 = call <vilib>:"Error Cluster From Error Code.vi"("show call chain? (False)"=TRUE, "error in (no error)"=w584, "error message (\"\")"=w585, "error code (0)"=w586) -> ("error out"=w583:errorcluster)  [unwired: 5 in]
        n222 = call <vilib>:"Add State(s) to Queue__jki_lib_state_machine.vi"("State(s) in (\"\")"=w581) -> ("States Out"=w580:string)  [unwired: 14 in]
      }
      frame "Initialize Core Data" {
        # "Do not delete, rename, or modify this frame.\n(this is used to determine panel behavior on exit)"
        # "originally closed?"
        # "exe?"
        # "If panel starts closed or is an EXE, then close it when we exit"
        n223 = property class="VI"() -> ("FP.State"=w592:T7)  [unwired: 2 in, 2 out]
        n224 = property class="App"() -> ("App.Kind"=w598:T8)  [unwired: 2 in, 2 out]
        n225 = control-ref of="Current VI Reference"() -> (w593:refnum<vi>)
        n226 = Equal?(x=w592, y=T7."Closed" ("Front Panel Window:State")) -> (x = y?=w590:bool)
        n227 = Equal?(x=w598, y=T8."Run Time System" ("Application:Kind")) -> (x = y?=w596:bool)
        n228 = Or(x=w590, y=w596) -> (x .or. y?=w594:bool)
        n229 = Bundle By Name(cluster=w595, "Core.Current VI Reference"=w593, "Core.Close Panel on Exit?"=w594) -> (w600:T25)
        n230 = call <vilib>:"Add State(s) to Queue__jki_lib_state_machine.vi"("State(s) in (\"\")"=w602) -> ("States Out"=w601:string)  [unwired: 14 in]
      }
      frame "Error Handler" {
        # "Unhandled Error -- Display it"
        # "Handle any errors here.\nYou can also output any states to clean-up after errors occur"
        # "Clear error"
        n231 = Unbundle By Name(w617) -> ("code"=w616:i32, "source"=w610:string)
        n232 = call <vilib>:"General Error Handler.vi"("error in (no error)"=w617) -> ()  [unwired: 10 in, 5 out]
        n233 = call <vilib>:"Search and Replace Pattern.vi"("string"=w610, "regular expression (\"\")"="\r", "replace all? (F)"=TRUE) -> ("result string"=w606:string)  [unwired: 2 in, 1 out]
        n234 = call <vilib>:"Search and Replace Pattern.vi"("string"=w606, "regular expression (\"\")"="\n") -> ("result string"=w605:string)  [unwired: 3 in, 1 out]
        n235 = Number To Decimal String(number=w616) -> (decimal integer string=w614:string)  [unwired: 1 in]
        n236 = call <vilib>:"Search and Replace Pattern.vi"("string"=w605, "regular expression (\"\")"="\r\n") -> ("result string"=w603:string)  [unwired: 3 in, 1 out]
        n237 = Concatenate Strings("ERROR{Error Code--" ("string"), w614, "--Error Source--" ("string"), w603, "}ERROR" ("string")) -> (w611:string)
        n238 = call <vilib>:"Add State(s) to Queue__jki_lib_state_machine.vi"("State(s) in Front (\"\")"="/* Post Error States", "State(s) in (\"\")"=w623) -> ("States Out"=w622:string)  [unwired: 13 in]
      }
      frame "Exit" {
        # "Do not put any code in this frame.\n(No errors that occur here will be handled.)"
        n239 = call <vilib>:"Add State(s) to Queue__jki_lib_state_machine.vi"("State(s) in (\"\")"=w629) -> ("States Out"=w628:string)  [unwired: 14 in]
      }
      frame "---------- Data ----------" {
        # "Do not put any code in this frame.\n(It is a separator no-op. You can make a copy of this frame to create a new Data frame)"
        n240 = call <vilib>:"Add State(s) to Queue__jki_lib_state_machine.vi"("State(s) in (\"\")"=w634) -> ("States Out"=w633:string)  [unwired: 14 in]
      }
      frame "Data: Status" {
        # "Data: Status\nInitialize the FGV with the name of the state for the status string"
        n241 = flat-sequence {
          tunnel: [w644] -> w636
          tunnel: w637 -> [w644]
          tunnel: [w642] -> _
          frame #0 {
            n242 = call "Status State.vi"("Status State In"="UI: Status", "Write"=TRUE) -> ("Status State Out"=w642:string)  [unwired: 3 in]
          }
        }
        n243 = call <vilib>:"Add State(s) to Queue__jki_lib_state_machine.vi"("State(s) in (\"\")"=w641) -> ("States Out"=w640:string)  [unwired: 14 in]
      }
      frame "Data: Initialize" {
        w646 = FALSE  # Cancel Archive
        w647 = path ""  # Archive Location
        w648 = cluster{"X":sgl, "Y":sgl}[] []  # Zoom History
        w649 = ""  # Offline Log
        w650 = refnum<class "Log.Litho.lvclass"> refnum  # log
        w651 = refnum<class "Inset.lvclass"> refnum  # inset
        w652 = T29 {"Hide Labels"=FALSE, "Image Data Range"={100.0, 0.0}, "Status"="", "Autosave Path"=path "", "Autosave?"=FALSE, "Inkscape File (.svg)"=path "", "Background Image"=path "", "Page"=0, "Normal Save Path"=path "", "Overwrite"=FALSE, "Pixellate?"=TRUE}  # UI
        w653 = path ""  # root path
        w656 = T30 []  # Litho
        w657 = T31 {"Paths"=[], "Rectangles"=[], "Background"=refnum, "Dots"=[], "Funnels"=[], "Other Images"=[]}  # Parsed Obj
        w658 = T32 {"Dots"=[], "Funnels"=[], "Rects"=[], "Paths"=[]}  # GUIDs
        w659 = T33 {"Path Changes"=[], "Funnel Changes"=[], "Rectangle Changes"=[], "Dot Changes"=[]}  # Changed Obj
        w660 = T34 {"Rectangles"=[], "Paths"=[], "Funnels"=[], "Dots"=[]}  # Obj Settings
        w662 = refnum<class "Configuration.lvclass"> refnum  # config
        w661 = refnum<class "AFM_Driver_Manager.lvclass"> refnum  # afm_mngr
        w665 = refnum<class "Selector.lvclass"> refnum  # selector
        w663 = refnum<class "BigMAQ.lvclass"> refnum  # big-maq
        w664 = refnum<class "Subpanel.Edit.lvclass"> refnum  # sbpnl.edit
        w668 = refnum<class "Tool Data.lvclass"> refnum  # tooler
        w666 = refnum<class "Setting Database.lvclass"> refnum  # settings
        w667 = refnum<class "ParseVectorFile.lvclass"> refnum  # parser
        w669 = T35 {"Current VI Reference"=refnum, "Close Panel on Exit?"=FALSE}  # Core
        # "do not delete - used by framework"
        # "Data names and types of shift register data are defined by this bundle."
        # "Initialize the shift-register data, here.\n(data names are defined by what you wire into the bundle function)"
        n244 = Bundle("Core"=w669, "tooler"=w668, "parser"=w667, "settings"=w666, "selector"=w665, "sbpnl.edit"=w664, "big-maq"=w663, "config"=w662, "afm_mngr"=w661, "Obj Settings"=w660, "Changed Obj"=w659, "GUIDs"=w658, "Parsed Obj"=w657, "Litho"=w656, "root path"=w653, "UI"=w652, "inset"=w651, "log"=w650, "Offline Log"=w649, "Zoom History"=w648, "Archive Location"=w647, "Cancel Archive"=w646) -> (w671:T25)  [unwired: 1 in]
        n245 = call <vilib>:"Add State(s) to Queue__jki_lib_state_machine.vi"("State(s) in (\"\")"=w673) -> ("States Out"=w672:string)  [unwired: 14 in]
      }
      frame "Data: Cleanup" {
        # "Cleanup any data and references, here.\n(this is called automatically, by the Macro: Exit)"
        n246 = Unbundle By Name(w675) -> ("Core.Current VI Reference"=w678:refnum<vi>)
        n247 = Close Reference(reference=w678, error in (no error)=w677) -> (error out=w676:errorcluster)
        n248 = call <vilib>:"Add State(s) to Queue__jki_lib_state_machine.vi"("State(s) in (\"\")"=w680) -> ("States Out"=w679:string)  [unwired: 14 in]
      }
      frame "---------- Events ----------" {
        # "Do not put any code in this frame.\n(It is a separator no-op. You can make a copy of this frame to create a new UI frame)"
        n249 = call <vilib>:"Add State(s) to Queue__jki_lib_state_machine.vi"("State(s) in (\"\")"=w685) -> ("States Out"=w684:string)  [unwired: 14 in]
      }
      frame "Events: Register" {
        # "Do not put any code in this frame.\n(It is a separator no-op. You can make a copy of this frame to create a new UI frame)"
        n250 = Unbundle By Name(w701) -> ("tooler"=w700:refnum<class "Tool Data.lvclass">, "parser"=w699:refnum<class "ParseVectorFile.lvclass">, "settings"=w698:refnum<class "Setting Database.lvclass">, "afm_mngr"=w689:refnum<class "AFM_Driver_Manager.lvclass">)
        n251 = call "AFM_Driver_Manager.GetPublicEvents.vi"("AFM_Driver_Manager in"=w689) -> ("error out"=w688:errorcluster, "AFM_Driver Events"=w687:T36)  [unwired: 8 in, 1 out]
        n252 = call "Setting Database.GetPublicEvents.vi"("Setting Database"=w698) -> ("error out"=w694:errorcluster, "Public Events"=w693:T37)  [unwired: 8 in, 1 out]
        n253 = call "ParseVectorFile.GetPublicEvents.vi"("ParseVectorFile"=w699) -> ("error out"=w695:errorcluster, "Public Events"=w692:T38)  [unwired: 8 in, 1 out]
        n254 = call "Tool Data.GetPublicEvents.vi"("Tool Data"=w700) -> ("error out"=w696:errorcluster, "Public Events"=w691:T39)  [unwired: 8 in, 1 out]
        n255 = register-events(w691, w692, w693, w687) -> (reference out=w703:refnum<event-registration>, error out=w702:errorcluster)  [unwired: 2 in]
        n256 = Merge Errors(w690, w702, w696, w695, w694, w688) -> (w697:errorcluster)
        n257 = call <vilib>:"Add State(s) to Queue__jki_lib_state_machine.vi"("State(s) in (\"\")"=w705) -> ("States Out"=w704:string)  [unwired: 14 in]
      }
      frame "Events: Unregister" {
        # "Do not put any code in this frame.\n(It is a separator no-op. You can make a copy of this frame to create a new UI frame)"
        n258 = Unregister For Events(event registration refnum=w709, error in=w708) -> (error out=w707:errorcluster)
        n259 = call <vilib>:"Add State(s) to Queue__jki_lib_state_machine.vi"("State(s) in (\"\")"=w712) -> ("States Out"=w711:string)  [unwired: 14 in]
      }
      frame "---------- UI ----------" {
        # "Do not put any code in this frame.\n(It is a separator no-op. You can make a copy of this frame to create a new UI frame)"
        n260 = call <vilib>:"Add State(s) to Queue__jki_lib_state_machine.vi"("State(s) in (\"\")"=w717) -> ("States Out"=w716:string)  [unwired: 14 in]
      }
      frame "UI: Tab Initialize" {
        # "Do not put any code in this frame.\n(It is a separator no-op. You can make a copy of this frame to create a new UI frame)"
        n261 = disable-structure shown="Default" {
          disable-tunnel: [T1."Home" ("NewVal") w764] -> w718
          frame condition #0 {
          }
          frame condition #1 (active) {
            n262 = local read "Tab Selectors"() -> (w764:T1)
          }
        }
        n263 = case shown="\"Home\"" w718 {
          selector: w718 -> [_ _ _ w756]
          tunnel: [u32 6316128 ("Boolean Text.Text Colors:Text Color") u32 6316128 ("Boolean Text.Text Colors:Text Color") u32 6316128 ("Boolean Text.Text Colors:Text Color") u32 2829099 ("Boolean Text.Text Colors:Text Color")] -> w727
          tunnel: [u32 6316128 ("Boolean Text.Text Colors:Text Color") u32 2829099 ("Boolean Text.Text Colors:Text Color") u32 6316128 ("Boolean Text.Text Colors:Text Color") u32 6316128 ("Boolean Text.Text Colors:Text Color")] -> w723
          tunnel: [u32 6316128 ("Boolean Text.Text Colors:Text Color") u32 6316128 ("Boolean Text.Text Colors:Text Color") u32 2829099 ("Boolean Text.Text Colors:Text Color") u32 6316128 ("Boolean Text.Text Colors:Text Color")] -> w721
          tunnel: [u32 2829099 ("Boolean Text.Text Colors:Text Color") u32 6316128 ("Boolean Text.Text Colors:Text Color") u32 6316128 ("Boolean Text.Text Colors:Text Color") u32 6316128 ("Boolean Text.Text Colors:Text Color")] -> w725
          tunnel: [T3."Patterns and Writing" ("Settings") T3."AFM Settings" ("Settings") T3."Image Settings" ("Settings") T3."Program Settings" ("Settings")] -> w719
          tunnel: [_ _ TRUE _] -> w720
          tunnel: [_ TRUE _ _] -> w722
          tunnel: [TRUE _ _ _] -> w724
          tunnel: [_ _ _ TRUE] -> w726
          frame "Patterns" {
          }
          frame "Microscope" {
          }
          frame "Image" {
          }
          frame "Home" {
            n264 = local write "Tab Selectors"(w756) -> ()
          }
        }
        n265 = local write "Settings"(w719) -> ()
        n266 = control-ref of="Home"() -> (w731:refnum<vi>)
        n267 = control-ref of="Patterns"() -> (w728:refnum<vi>)
        n268 = control-ref of="Microscope"() -> (w730:refnum<vi>)
        n269 = control-ref of="Image"() -> (w729:refnum<vi>)
        n270 = property class="Bool (strict)"(reference=w731, "BoolText.TextColor"=w727, "BoolText.FontBold"=w726) -> ()  [unwired: 1 in, 2 out]
        n271 = property class="Bool (strict)"(reference=w728, "BoolText.TextColor"=w725, "BoolText.FontBold"=w724) -> ()  [unwired: 1 in, 2 out]
        n272 = property class="Bool (strict)"(reference=w730, "BoolText.TextColor"=w723, "BoolText.FontBold"=w722) -> ()  [unwired: 1 in, 2 out]
        n273 = property class="Bool (strict)"(reference=w729, "BoolText.TextColor"=w721, "BoolText.FontBold"=w720) -> ()  [unwired: 1 in, 2 out]
        n274 = call <vilib>:"Add State(s) to Queue__jki_lib_state_machine.vi"("State(s) in (\"\")"=w737) -> ("States Out"=w736:string)  [unwired: 14 in]
      }
      frame "UI: Create Insert" {
        # "Do not put any code in this frame.\n(It is a separator no-op. You can make a copy of this frame to create a new UI frame)"
        n275 = Unbundle By Name(w794) -> ("inset"=w789:refnum<class "Inset.lvclass">, "UI.Image Data Range"=w787:cluster{sgl, sgl}, "UI.Page"=w786:u32, "big-maq"=w771:refnum<class "BigMAQ.lvclass">, "UI.Inkscape File (.svg)"=w784:path, "Parsed Obj.Background"=w783:refnum<class "SVGImage.lvclass">)
        n276 = Bundle(cluster=T9 {"Background.Range"={0.0, 100.0}, "Background.Page"=0} ("Display Settings"), "Background.Range"=w787, "Background.Page"=w786) -> (w785:T9)
        n277 = call "Setup Background BigMAQ.vi"("error in"=w778, "BigMAQ"=w771, "Display Settings"=w785, "Inset in"=w789) -> ("error out"=w781:errorcluster, "Inset out"=w793:refnum<class "Inset.lvclass">)  [unwired: 6 in]
        n278 = call "Write SVG Path.vi"("error in"=w781, "Path"=w784, "Inset in"=w793) -> ("error out"=w780:errorcluster, "Inset out"=w792:refnum<class "Inset.lvclass">)  [unwired: 7 in]
        n279 = call-dynamic "Read id.vi"("error in (no error)"=w780, "SVG Object in"=w783) -> ("error out"=w779:errorcluster, "id"=w782:string)  [unwired: 7 in, 1 out]
        n280 = call "Set Background id.vi"("error in"=w779, "id"=w782, "Inset in"=w792) -> ("error out"=w790:errorcluster, "Inset out"=w791:refnum<class "Inset.lvclass">)  [unwired: 7 in]
        n281 = call "User Interface.vi"("error in"=w790, "Inset In"=w791) -> ("error out"=w775:errorcluster, "Inset Out"=w777:refnum<class "Inset.lvclass">)  [unwired: 8 in]
        n282 = call "Get Background Settings.vi"("error in"=w775, "BigMAQ"=w771, "Inset in"=w777) -> ("error out"=w774:errorcluster, "Background.Page"=w772:i32, "Background.Range"=w773:cluster{sgl, sgl}, "Inset out"=w776:refnum<class "Inset.lvclass">, "status"=w770:bool)  [unwired: 4 in]
        n283 = Bundle By Name(cluster=w794, "inset"=w776, "UI.Image Data Range"=w773, "UI.Page"=w772) -> (w795:T25)
        n284 = Select(t="Big MAQ: Initialize\nUI: Big MAQ Initialize\nBig MAQ: Read Background", s=w770, f="") -> (s? t:f=w765:string)
        n285 = call <vilib>:"Add State(s) to Queue__jki_lib_state_machine.vi"("State(s) in (\"\")"=w765, "State(s) at Back (\"\")"="UI: Update Control >> Image Data Range\nUI: Update Control>>Page\nBig MAQ: Select Page\nBig MAQ: Change Data Range\nBig MAQ: Generate Overlay\nBig MAQ: Update" ("State(s) in Front (\"\")")) -> ("States Out"=w767:string)  [unwired: 13 in]
        n286 = call <vilib>:"Add State(s) to Queue__jki_lib_state_machine.vi"("State(s) in Front (\"\")"=w767, "State(s) in (\"\")"=w799) -> ("States Out"=w798:string)  [unwired: 13 in]
      }
      frame "UI: Update Zoom Factor" {
        # "Do not put any code in this frame.\n(It is a separator no-op. You can make a copy of this frame to create a new UI frame)"
        n287 = control-ref of="Render"() -> (w804:refnum<vi>)
        n288 = property class="ImageControl"(reference=w804) -> ("X Zoom"=w800:sgl)  [unwired: 1 in, 2 out]
        n289 = Format Into String(format string="%3.1f", initial string="", w800) -> (resulting string=w807:string)  [unwired: 1 in, 1 out]
        n290 = Concatenate Strings(w807, "x" ("string")) -> (w803:string)
        n291 = local write "Zoom"(w803) -> ()
        n292 = call <vilib>:"Add State(s) to Queue__jki_lib_state_machine.vi"("State(s) in (\"\")"=w812) -> ("States Out"=w811:string)  [unwired: 14 in]
      }
      frame "UI: Select Initialize" {
        # "Do not put any code in this frame.\n(It is a separator no-op. You can make a copy of this frame to create a new UI frame)"
        n293 = Unbundle By Name(w816) -> ("selector"=w815:refnum<class "Selector.lvclass">)
        n294 = call "UI--Initialize.vi"("error in"=w817, "Selector in"=w815) -> ("error out"=w818:errorcluster, "Selector out"=w814:refnum<class "Selector.lvclass">)  [unwired: 8 in]
        n295 = Bundle By Name(cluster=w816, "selector"=w814) -> (w819:T25)
        n296 = call <vilib>:"Add State(s) to Queue__jki_lib_state_machine.vi"("State(s) in (\"\")"=w822) -> ("States Out"=w821:string)  [unwired: 14 in]
      }
      frame "UI: Enable Run" {
        # "Do not put any code in this frame.\n(It is a separator no-op. You can make a copy of this frame to create a new UI frame)"
        n297 = Match True/False String(2:"Disabled" ("false string"), 3:"Enabled" ("true string"), 4:w826) -> (0:w833:bool)  [unwired: 1 out]
        n298 = Select(t=T10."Enabled" ("Disabled"), s=w833, f=T10."Disabled and Grayed Out" ("Disabled")) -> (s? t:f=w832:T10)
        n299 = control-ref of="Run"() -> (w827:refnum<vi>)
        n300 = property class="Bool (strict)"(reference=w827, error in=w824, "DisabledEnum"=w832) -> (error out=w825:errorcluster)  [unwired: 1 out]
        n301 = call <vilib>:"Add State(s) to Queue__jki_lib_state_machine.vi"("State(s) in (\"\")"=w837) -> ("States Out"=w836:string)  [unwired: 14 in]
      }
      frame "UI: Status" {
        # "This must be empty string otherwise you will get stuck"
        # "Do not put any code in this frame.\n(It is a separator no-op. You can make a copy of this frame to create a new UI frame)"
        n302 = Unbundle By Name(w849) -> ("UI.Status"=w841:string, "log"=w842:refnum<class "Log.Litho.lvclass">)
        n303 = call <vilib>:"GetState.vi"("error in (no error)"=w847, "SMO"=w842) -> ("error out"=w845:errorcluster, "SMO State"=w848:T40, "SMO out"=w846:refnum<class "Log.Litho.lvclass">)  [unwired: 7 in]
        n304 = call "Status Append.vi"("New Status In"=w838, "Status Log In"=w841) -> ("Status Log Out"=w839:string, "Time Stamped Status String"=w840:string)  [unwired: 1 in, 1 out]
        n305 = case shown="\"Started\"" w848 {
          tunnel: w846 -> [w860 w865]
          tunnel: w845 -> [w859 w862]
          tunnel: w840 -> [w856 w861]
          tunnel: [w858 w864] -> w843
          tunnel: [w857 w863] -> w844
          frame Default {
            n306 = call <vilib>:"Clear Errors.vi"("error in (no error)"=w859) -> ("error out"=w855:errorcluster)  [unwired: 5 in, 1 out]
            n307 = call-dynamic "Write Offline Log.vi"("error in (no error)"=w855, "Offline Log"=w856, "Log.Litho in"=w860) -> ("error out"=w857:errorcluster, "Log.Litho out"=w858:refnum<class "Log.Litho.lvclass">)  [unwired: 7 in]
          }
          frame "Started" {
            n308 = call "Log.Litho.Activity.vi"("error in (no error)"=w862, "Activity"=w861, "Log.Litho"=w865) -> ("error out"=w863:errorcluster, "Log.Litho out"=w864:refnum<class "Log.Litho.lvclass">)  [unwired: 7 in]
          }
        }
        n309 = local write "Status"(w839) -> ()
        n310 = Bundle By Name(cluster=w849, "UI.Status"=w839, "log"=w843) -> (w851:T25)
        n311 = call <vilib>:"Add State(s) to Queue__jki_lib_state_machine.vi"("State(s) in (\"\")"=w854) -> ("States Out"=w853:string)  [unwired: 14 in]
      }
      frame "UI: Big MAQ Initialize" {
        # "Do not put any code in this frame.\n(It is a separator no-op. You can make a copy of this frame to create a new UI frame)"
        n312 = Unbundle By Name(w873) -> ("big-maq"=w875:refnum<class "BigMAQ.lvclass">)
        n313 = call "Initialize UI.vi"("error in"=w872, "BigMAQ in"=w875) -> ("error out"=w868:errorcluster, "BigMAQ out"=w870:refnum<class "BigMAQ.lvclass">)  [unwired: 8 in]
        n314 = call-dynamic "Read Voltage Scale.vi"("error in (no error)"=w868, "BigMAQ in"=w870) -> ("error out"=w867:errorcluster, "Voltage Scale"=w866:dbl, "BigMAQ out"=w869:refnum<class "BigMAQ.lvclass">)  [unwired: 7 in]
        n315 = local write "Voltage Color Scale"(w866) -> ()
        n316 = Bundle By Name(cluster=w873, "big-maq"=w869) -> (w874:T25)
        n317 = call <vilib>:"Add State(s) to Queue__jki_lib_state_machine.vi"("State(s) in (\"\")"=w878) -> ("States Out"=w877:string)  [unwired: 14 in]
      }
      frame "UI: Update Control" {
        n318 = call <vilib>:"Parse State Queue__jki_lib_state_machine.vi"("State Queue"=w881, "Error In (no error)"=w883) -> ("Current State"=w882:string, "Arguments"=w880:string)  [unwired: 11 in, 1 out]
        n319 = case shown="\"Overwrite\"" w882 {
          tunnel: w889 -> [w893 w899 w902 w907 w912 w917 w924 w933 w938 w941 w947 w950 w956]
          tunnel: [w893 w899 w902 w907 w912 w917 w924 w933 w938 w941 w947 w950 w956] -> w888
          tunnel: w886 -> [w895 w898 w904 w909 w914 w919 w923 w932 w937 w943 w945 w953 w958]
          tunnel: [w895 w898 w904 w909 w914 w919 w923 w932 w937 w943 w945 w953 w958] -> w887
          tunnel: w883 -> [w894 w897 w903 w908 w913 w918 w922 w931 w936 w942 w948 w952 w957]
          tunnel: [w894 w897 w903 w908 w913 w918 w922 w931 w936 w942 w948 w952 w957] -> w885
          tunnel: w880 -> [_ _ _ _ _ _ w920 w928 w935 _ _ _ _]
          tunnel: ["Normal Render Save Path Control Updated" "" "Autosave Render Overwrite Control Updated" "Image Data Range Updated via Program" "Autosave Path Control Updated" "Autosave Boolean Updated" "" "Ready Updated" "Image Filename Indicator Updated" "Background Image Control Updated" "Inkscape File Path Control Updated" "Hide Labels Control Updated" "Page Control Updated via Program"] -> w879
          frame "Normal Save Path" {
            n320 = Unbundle By Name(w893) -> ("UI.Normal Save Path"=w892:path)
            n321 = local write "Normal Save Path"(w892) -> ()
          }
          frame Default {
          }
          frame "Overwrite" {
            n322 = Unbundle By Name(w902) -> ("UI.Overwrite"=w901:bool)
            n323 = local write "Overwrite?"(w901) -> ()
          }
          frame "Image Data Range" {
            n324 = Unbundle By Name(w907) -> ("UI.Image Data Range"=w906:cluster{sgl, sgl})
            n325 = local write "Image Data Range"(w906) -> ()
          }
          frame "Autosave Path" {
            n326 = Unbundle By Name(w912) -> ("UI.Autosave Path"=w911:path)
            n327 = local write "Autosave Path"(w911) -> ()
          }
          frame "Autosave" {
            n328 = Unbundle By Name(w917) -> ("UI.Autosave?"=w916:bool)
            n329 = local write "Autosave?"(w916) -> ()
          }
          frame "Estimated Time" {
            n330 = local write "Estimated Time"(w920) -> ()
          }
          frame "Ready" {
            n331 = To Upper Case(1:w928) -> (0:w926:string)
            n332 = Match True/False String(2:"FALSE" ("false string"), 3:"TRUE" ("true string"), 4:w926) -> (0:w927:bool)  [unwired: 1 out]
            n333 = local write "Ready?"(w927) -> ()
          }
          frame "Image Filename" {
            n334 = local write "Image Filename"(w935) -> ()
          }
          frame "Background Image" {
            # "UI: Update Control >>Background Image"
            n335 = Unbundle By Name(w941) -> ("UI.Background Image"=w940:path)
            n336 = local write "Background Image"(w940) -> ()
          }
          frame "Inkscape" {
            n337 = Unbundle By Name(w947) -> ("UI.Inkscape File (.svg)"=w946:path)
            n338 = local write "Inkscape File (.svg)"(w946) -> ()
          }
          frame "Hide Labels" {
            n339 = Unbundle By Name(w950) -> ("UI.Hide Labels"=w951:bool)
            n340 = local write "Hide Labels?"(w951) -> ()
          }
          frame "Page" {
            n341 = Unbundle By Name(w956) -> ("UI.Page"=w955:u32)
            n342 = local write "Data Channel"(w955) -> ()
          }
        }
        n343 = call <vilib>:"Add State(s) to Queue__jki_lib_state_machine.vi"("State(s) in (\"\")"=w887) -> ("States Out"=w890:string)  [unwired: 14 in]
      }
      frame "UI: Initialize" {
        # "Initialize the User Interface, here.\n(this is called automatically, by the Macro: Init)"
        n344 = Unbundle By Name(w974) -> ("Core.Current VI Reference"=w959:refnum<vi>)
        n345 = control-ref of="Status"() -> (w978:refnum<vi>)
        n346 = call <userlib>:"MGI Get Executable Version.vi"() -> ("Version"=w973:string)  [unwired: 7 in]
        n347 = control-ref of="Overwrite?"() -> (w961:refnum<vi>)
        n348 = property class="Bool (strict)"(reference=w961, "Visible"=TRUE) -> ()  [unwired: 1 in, 2 out]
        n349 = Concatenate Strings("v" ("string"), w973, "_beta" ("string")) -> (w972:string)
        n350 = property class="Str"(reference=w978, error in=w975, "Text.FontName"="Consolas" ("Text.Font:Name"), "Text.FontSize"=u32 20 ("Text.Font:Size")) -> (error out=w967:errorcluster)  [unwired: 1 out]
        n351 = control-ref of="Type:"() -> (w969:refnum<vi>)
        n352 = local write "version"(w972) -> ()
        n353 = property class="Ring (strict)"(reference=w969, error in=w967, "Strings []"=string[] ["Asylum"] ("t")) -> (error out=w966:errorcluster)  [unwired: 1 out]
        n354 = local write "Image Data Range"(cluster{sgl, sgl} {100.0, 0.0} ("Image Data Range")) -> ()
        n355 = call <userlib>:"Fit VI window to Largest Dec__ogtk.vi"("error in (no error)"=w966, "VI Ref (calling VI)"=w959) -> ("error out"=w963:errorcluster)  [unwired: 4 in, 1 out]
        n356 = flat-sequence {
          tunnel: w963 -> [w986]
          tunnel: [w986] -> w962
          frame #0 {
            n357 = local write "Archive"(FALSE ("Archive")) -> ()
            n358 = local write "Unarchive"(FALSE ("Unarchive")) -> ()
            n359 = local write "Abort"(FALSE ("Abort")) -> ()
            n360 = local write "Help"(FALSE ("Help")) -> ()
            n361 = local write "Done"(FALSE ("Done")) -> ()
            n362 = local write "Refresh Button"(FALSE ("Refresh Button")) -> ()
            n363 = local write "Run"(FALSE ("Run")) -> ()
            n364 = local write "Slow Alert"(TRUE ("Slow Alert")) -> ()
            n365 = local write "Pixellate?"(TRUE ("Pixellate?")) -> ()
          }
        }
        n366 = call <vilib>:"Add State(s) to Queue__jki_lib_state_machine.vi"("State(s) in (\"\")"=w981) -> ("States Out"=w980:string)  [unwired: 14 in]
      }
      frame "UI: Cursor Set" {
        # "Argument"
        # "Set and Unset Cursor Busy.\n(Usage: \"UI: Cursor Set >> Busy|Idle\")"
        n367 = case shown="\"Idle\", Default" w993 {
          tunnel: w995 -> [w1000 w1002]
          tunnel: [w999 w1001] -> w994
          frame "Idle", Default {
            n368 = call <vilib>:"Unset Busy.vi"("error in (no error)"=w1000) -> ("error out"=w999:errorcluster)  [unwired: 10 in]
          }
          frame "Busy" {
            n369 = call <vilib>:"Set Busy.vi"("error in (no error)"=w1002) -> ("error out"=w1001:errorcluster)  [unwired: 9 in, 1 out]
          }
        }
        n370 = call <vilib>:"Add State(s) to Queue__jki_lib_state_machine.vi"("State(s) in (\"\")"=w998) -> ("States Out"=w997:string)  [unwired: 14 in]
      }
      frame "UI: Front Panel State" {
        # "Argument"
        # "Set Front Panel Open or Closed\n(Usage: \"UI: Front Panel State >> Open|Close\")"
        n371 = Unbundle By Name(w1006) -> ("Core.Current VI Reference"=w1005:refnum<vi>)
        n372 = case shown="\"Open\", \"Standard\", Default" w1004 {
          tunnel: w1008 -> [w1016 w1031 w1042 w1055 w1068]
          tunnel: [w1018 w1032 w1044 w1057 w1070] -> w1007
          tunnel: w1005 -> [w1017 w1029 w1043 w1056 w1069]
          frame "Open", "Standard", Default {
            w1011 = T7."Standard" ("State")
            n373 = property class="VI"(reference=w1017, error in=w1016) -> (reference out=w1014:refnum<vi>, error out=w1015:errorcluster, "FP.State"=w1013:T7)
            n374 = Not Equal?(x=w1013, y=w1011) -> (x != y?=w1012:bool)
            n375 = case shown="False" w1012 {
              tunnel: [w1022 w1024] -> w1018
              tunnel: w1015 -> [w1021 w1024]
              tunnel: w1014 -> [w1020 _]
              tunnel: w1011 -> [w1019 _]
              frame True {
                n376 = invoke class="VI" method="FP.Open"(reference=w1020, error in=w1021, "Activate"=TRUE, "State"=w1019) -> (error out=w1022:errorcluster)  [unwired: 1 in, 4 out]
              }
              frame False {
              }
            }
          }
          frame "Close", "Closed" {
            n377 = property class="VI"(reference=w1029, error in=w1031) -> (reference out=w1028:refnum<vi>, error out=w1030:errorcluster, "FP.State"=w1026:T7)
            n378 = Not Equal?(x=w1026, y=T7."Closed" ("Front Panel Window:State")) -> (x != y?=w1025:bool)
            n379 = case shown="True" w1025 {
              tunnel: [w1033 w1036] -> w1032
              tunnel: w1030 -> [w1033 w1035]
              tunnel: w1028 -> [_ w1034]
              frame False {
              }
              frame True {
                n380 = invoke class="VI" method="FP.Close"(reference=w1034, error in=w1035) -> (error out=w1036:errorcluster)  [unwired: 1 in, 2 out]
              }
            }
          }
          frame "Hidden", "Hide" {
            w1037 = T7."Hidden" ("State")
            n381 = property class="VI"(reference=w1043, error in=w1042) -> (reference out=w1040:refnum<vi>, error out=w1041:errorcluster, "FP.State"=w1039:T7)
            n382 = Not Equal?(x=w1039, y=w1037) -> (x != y?=w1038:bool)
            n383 = case shown="True" w1038 {
              tunnel: [w1048 w1049] -> w1044
              tunnel: w1041 -> [w1047 w1049]
              tunnel: w1040 -> [w1046 _]
              tunnel: w1037 -> [w1045 _]
              frame True {
                n384 = invoke class="VI" method="FP.Open"(reference=w1046, error in=w1047, "State"=w1045) -> (error out=w1048:errorcluster)  [unwired: 2 in, 4 out]
              }
              frame False {
              }
            }
          }
          frame "Minimize", "Minimized" {
            w1050 = T7."Minimized" ("State")
            n385 = property class="VI"(reference=w1056, error in=w1055) -> (reference out=w1053:refnum<vi>, error out=w1054:errorcluster, "FP.State"=w1052:T7)
            n386 = Not Equal?(x=w1052, y=w1050) -> (x != y?=w1051:bool)
            n387 = case shown="True" w1051 {
              tunnel: [w1061 w1062] -> w1057
              tunnel: w1054 -> [w1060 w1062]
              tunnel: w1053 -> [w1059 _]
              tunnel: w1050 -> [w1058 _]
              frame True {
                n388 = invoke class="VI" method="FP.Open"(reference=w1059, error in=w1060, "State"=w1058) -> (error out=w1061:errorcluster)  [unwired: 2 in, 4 out]
              }
              frame False {
              }
            }
          }
          frame "Maximize", "Maximized" {
            w1063 = T7."Maximized" ("State")
            n389 = property class="VI"(reference=w1069, error in=w1068) -> (reference out=w1066:refnum<vi>, error out=w1067:errorcluster, "FP.State"=w1065:T7)
            n390 = Not Equal?(x=w1065, y=w1063) -> (x != y?=w1064:bool)
            n391 = case shown="True" w1064 {
              tunnel: [w1074 w1075] -> w1070
              tunnel: w1067 -> [w1073 w1075]
              tunnel: w1066 -> [w1072 _]
              tunnel: w1063 -> [w1071 _]
              frame True {
                n392 = invoke class="VI" method="FP.Open"(reference=w1072, error in=w1073, "State"=w1071) -> (error out=w1074:errorcluster)  [unwired: 2 in, 4 out]
              }
              frame False {
              }
            }
          }
        }
        n393 = call <vilib>:"Add State(s) to Queue__jki_lib_state_machine.vi"("State(s) in (\"\")"=w1010) -> ("States Out"=w1009:string)  [unwired: 14 in]
      }
      frame "---------- Macro ----------" {
        # "Do not put any code in this frame.\n(It is a separator no-op. You can make a copy of this frame to create a new Macro frame)"
        n394 = call <vilib>:"Add State(s) to Queue__jki_lib_state_machine.vi"("State(s) in (\"\")"=w1080) -> ("States Out"=w1079:string)  [unwired: 14 in]
      }
      frame "Macro: Start SMOs" {
        # "Do not put any code in this frame.\n(It is a separator no-op. You can make a copy of this frame to create a new Macro frame)"
        n395 = call <vilib>:"Add State(s) to Queue__jki_lib_state_machine.vi"("State(s) in Front (\"\")"="Tool: Start\nSettings: Start\nSubpanel: Initialize //This also has SMOs in it for the subpanels\nParse: Start", "State(s) in (\"\")"=w1086) -> ("States Out"=w1085:string)  [unwired: 13 in]
      }
      frame "Macro: Start Subsystems" {
        # "Do not put any code in this frame.\n(It is a separator no-op. You can make a copy of this frame to create a new Macro frame)"
        n396 = call <vilib>:"Add State(s) to Queue__jki_lib_state_machine.vi"("State(s) in Front (\"\")"="Select: Create\nBig MAQ: Initialize", "State(s) in (\"\")"=w1092) -> ("States Out"=w1091:string)  [unwired: 13 in]
      }
      frame "Macro: Initialize UI" {
        # "Do not put any code in this frame.\n(It is a separator no-op. You can make a copy of this frame to create a new Macro frame)"
        n397 = call <vilib>:"Add State(s) to Queue__jki_lib_state_machine.vi"("State(s) in Front (\"\")"="UI: Initialize\nUI: Tab Initialize\nUI: Enable Run >> Enabled\nUI: Big MAQ Initialize\nUI: Select Initialize\nUI: Update Control >> Hide Labels\nUI: Front Panel State >> Open", "State(s) in (\"\")"=w1098) -> ("States Out"=w1097:string)  [unwired: 13 in]
      }
      frame "Macro: Objects Updated" {
        # "Do not put any code in this frame.\n(It is a separator no-op. You can make a copy of this frame to create a new Macro frame)"
        n398 = call <vilib>:"Add State(s) to Queue__jki_lib_state_machine.vi"("State(s) in Front (\"\")"="UI: Update Control >> Ready >> False\nSelect: Apply Symbols\nSelect: Update\nTool: Objects" ("State(s) in Front (\"\")"), "State(s) in (\"\")"=w1104) -> ("States Out"=w1103:string)  [unwired: 13 in]
      }
      frame "Macro: Initialize" {
        # "Initialization Macro\n(This is called once, when the VI starts)"
        n399 = call <vilib>:"Add State(s) to Queue__jki_lib_state_machine.vi"("State(s) in Front (\"\")"="Data: Initialize\nInitialize Core Data\nData: Status //needs to be initialized really early\nLog: Start\nUI: Update Control >> Ready >> False\nFile: Get Root Path\nConfig: Initialize\nConfig: Read\nUI: Update Control >> Autosave Path\nUI: Update Control >> Autosave\nUI: Update Control >> Overwrite\nUI: Update Control >> Normal Save Path\n//File: Get Control Values\nAFM: Initialize Manager\nAFM: Initialize Driver\nAFM: Set Active >> 0\nAFM: Insert Into Subpanel\nMacro: Start SMOs\nEvents: Register\nMacro: Start Subsystems\nMacro: Initialize UI\nFile: Inkscape\nFile: Background\nAFM: Background Image\nBig MAQ: Read Background\nBig MAQ: Update\nBig MAQ: Zoom Fit\nBig MAQ: Save Background\nUI: Update Zoom Factor\nParse: Send File // this event will kick everything else off", "State(s) in (\"\")"=w1110) -> ("States Out"=w1109:string)  [unwired: 13 in]
      }
      frame "Macro: Exit" {
        # "Exit Macro\n(This is called once, when the VI exits)"
        n400 = Unbundle By Name(w1118) -> ("Core.Close Panel on Exit?"=w1117:bool)
        n401 = Select(t="UI: Front Panel State >> Close", s=w1117, f="") -> (s? t:f=w1114:string)
        n402 = call <vilib>:"Add State(s) to Queue__jki_lib_state_machine.vi"("State(s) in (\"\")"=w1114, "State(s) at Back (\"\")"="Config: Write\nAFM: Stop Manager\nParse: Stop\nSubpanel: Close\nSettings: Stop\nTool: Stop\nBig MAQ: Cleanup\nIdentity: Destroy Registry\nLog: Stop\nData: Cleanup\nEvents: Unregister\nExit") -> ("States Out"=w1112:string)  [unwired: 13 in]
        n403 = call <vilib>:"Add State(s) to Queue__jki_lib_state_machine.vi"("State(s) in Front (\"\")"=w1112, "State(s) in (\"\")"=w1121) -> ("States Out"=w1120:string)  [unwired: 13 in]
      }
      frame "---------- File ----------" {
        # "Do not put any code in this frame.\n(It is a separator no-op. You can make a copy of this frame to create a new UI frame)"
        n404 = call <vilib>:"Add State(s) to Queue__jki_lib_state_machine.vi"("State(s) in (\"\")"=w1126) -> ("States Out"=w1125:string)  [unwired: 14 in]
      }
      frame "File: Get Control Values" {
        # "Do not put any code in this frame.\n(It is a separator no-op. You can make a copy of this frame to create a new UI frame)"
        n405 = local read "Background Image"() -> (w1129:path)
        n406 = local read "Inkscape File (.svg)"() -> (w1127:path)
        n407 = local read "Autosave Path"() -> (w1128:path)
        n408 = Bundle By Name(cluster=w1130, "UI.Inkscape File (.svg)"=w1127, "UI.Background Image"=w1129, "UI.Autosave Path"=w1128) -> (w1131:T25)
        n409 = call <vilib>:"Add State(s) to Queue__jki_lib_state_machine.vi"("State(s) in (\"\")"=w1135) -> ("States Out"=w1134:string)  [unwired: 14 in]
      }
      frame "File: Get Root Path" {
        # "Do not put any code in this frame.\n(It is a separator no-op. You can make a copy of this frame to create a new UI frame)"
        n410 = call <userlib>:"Current VI's Path__ogtk.vi"() -> ("Current VI's Path (+ Relative)"=w1139:path)  [unwired: 1 in]
        n411 = Strip Path(path=w1139) -> (stripped path=w1138:path)  [unwired: 1 out]
        n412 = Bundle By Name(cluster=w1136, "root path"=w1138) -> (w1137:T25)
        n413 = call <vilib>:"Add State(s) to Queue__jki_lib_state_machine.vi"("State(s) in (\"\")"=w1143) -> ("States Out"=w1142:string)  [unwired: 14 in]
      }
      frame "File: Autosave Path" {
        # "Do not put any code in this frame.\n(It is a separator no-op. You can make a copy of this frame to create a new UI frame)"
        n414 = call <vilib>:"Add State(s) to Queue__jki_lib_state_machine.vi"("State(s) in (\"\")"=w1148) -> ("States Out"=w1147:string)  [unwired: 14 in]
      }
      frame "File: Inkscape" {
        # "Do not put any code in this frame.\n(It is a separator no-op. You can make a copy of this frame to create a new UI frame)"
        n415 = Unbundle By Name(w1152) -> ("UI.Inkscape File (.svg)"=w1164:path)
        n416 = call "CheckFileConformity.vi"("error in (no error)"=w1157, "File Data"=T11 {"Pattern"="svg", "Pattern Label"="Scalable Vector Graphics", "Prompt"="Choose an SVG file"}, "Path In"=w1164) -> ("error out"=w1162:errorcluster, "No File"=w1159:bool, "Path Out"=w1163:path, "Asked to Change?"=w1156:bool)  [unwired: 5 in]
        n417 = case shown="True" w1159 {
          tunnel: w1163 -> [w1169 _]
          tunnel: w1162 -> [w1168 w1172]
          tunnel: [w1168 w1174] -> w1158
          tunnel: [w1169 w1173] -> w1161
          frame False {
          }
          frame True {
            n418 = call "Display Message to User2"("error in (no error)"=w1172, "Message"="No Valid File Selected. Using Default.") -> ("error out"=w1171:errorcluster)  [unwired: 8 in, 1 out]
            n419 = call "GenerateDefaultSVGFile.vi"("error in (no error)"=w1171) -> ("error out"=w1174:errorcluster, "Path"=w1173:path)  [unwired: 9 in]
          }
        }
        n420 = Select(t="", s=w1156, f="Config: Write") -> (s? t:f=w1150:string)
        n421 = Bundle By Name(cluster=w1152, "UI.Inkscape File (.svg)"=w1161) -> (w1153:T25)
        n422 = call <vilib>:"Add State(s) to Queue__jki_lib_state_machine.vi"("State(s) in Front (\"\")"=w1150, "State(s) in (\"\")"="UI: Update Control >> Inkscape" ("State(s) at Back (\"\")")) -> ("States Out"=w1149:string)  [unwired: 13 in]
        n423 = call <vilib>:"Add State(s) to Queue__jki_lib_state_machine.vi"("State(s) in Front (\"\")"=w1149, "State(s) in (\"\")"=w1167) -> ("States Out"=w1166:string)  [unwired: 13 in]
      }
      frame "File: Background" {
        # "Do not put any code in this frame.\n(It is a separator no-op. You can make a copy of this frame to create a new UI frame)"
        n424 = Unbundle By Name(w1189) -> ("UI.Background Image"=w1195:path)
        n425 = call "CheckFileConformity.vi"("error in (no error)"=w1188, "File Data"=T11 {"Pattern"="ibw", "Pattern Label"="Igor Binary Wave", "Prompt"="Choose an IBW file"}, "Path In"=w1195) -> ("error out"=w1192:errorcluster, "No File"=w1191:bool, "Path Out"=w1193:path, "Asked to Change?"=w1187:bool)  [unwired: 5 in]
        n426 = case shown="True" w1191 {
          tunnel: w1192 -> [w1199 w1202]
          tunnel: w1193 -> [w1200 _]
          tunnel: [w1200 w1204] -> w1184
          tunnel: [w1199 w1205] -> w1182
          frame False {
          }
          frame True {
            n427 = call "Display Message to User"("error in (no error)"=w1202, "Message"="No Valid File Selected. Using Default.") -> ("error out"=w1201:errorcluster)  [unwired: 8 in, 1 out]
            n428 = call "GenerateDefaultIBWFile.vi"("error in (no error)"=w1201) -> ("error out"=w1205:errorcluster, "Path"=w1204:path)  [unwired: 9 in]
          }
        }
        n429 = Select(t="", s=w1187, f="Config: Write") -> (s? t:f=w1177:string)
        n430 = call <vilib>:"Get File Extension.vi"("error in (no error)"=w1182, "file"=w1184) -> ("error out"=w1181:errorcluster, "filename without extension"=w1180:string, "dup file"=w1183:path)  [unwired: 5 in, 2 out]
        n431 = call <vilib>:"Build State String with Arguments__JKI_lib_State_Machine.vi"("Arguments (\"\")"=w1180, "State"="UI: Update Control >> Image Filename") -> ("State with Arguments"=w1175:string)  [unwired: 4 in]
        n432 = Bundle By Name(cluster=w1189, "UI.Background Image"=w1183) -> (w1190:T25)
        n433 = call <vilib>:"Add State(s) to Queue__jki_lib_state_machine.vi"("State(s) in Front (\"\")"=w1177, "State(s) in (\"\")"="UI: Update Control >> Background Image" ("State(s) at Back (\"\")"), "State(s) at Back (\"\")"=w1175) -> ("States Out"=w1179:string)  [unwired: 12 in]
        n434 = call <vilib>:"Add State(s) to Queue__jki_lib_state_machine.vi"("State(s) in Front (\"\")"=w1179, "State(s) in (\"\")"=w1198) -> ("States Out"=w1197:string)  [unwired: 13 in]
      }
      frame "---------- Identity ----------" {
        # "Do not put any code in this frame.\n(It is a separator no-op. You can make a copy of this frame to create a new UI frame)"
        n435 = call <vilib>:"Add State(s) to Queue__jki_lib_state_machine.vi"("State(s) in (\"\")"=w1210) -> ("States Out"=w1209:string)  [unwired: 14 in]
      }
      frame "Identity: Destroy Registry" {
        # "Do not put any code in this frame.\n(It is a separator no-op. You can make a copy of this frame to create a new UI frame)"
        n436 = call "Destroy Registry.vi"("error in"=w1212) -> ("error out"=w1213:errorcluster)  [unwired: 10 in]
        n437 = call <vilib>:"Add State(s) to Queue__jki_lib_state_machine.vi"("State(s) in (\"\")"=w1217) -> ("States Out"=w1216:string)  [unwired: 14 in]
      }
      frame "Identity: Populate" {
        # "Do not put any code in this frame.\n(It is a separator no-op. You can make a copy of this frame to create a new UI frame)"
        n438 = Unbundle By Name(w1226) -> ("GUIDs.Dots"=w1223:string[], "GUIDs.Funnels"=w1222:string[], "GUIDs.Rects"=w1221:string[], "GUIDs.Paths"=w1224:string[])
        n439 = Bundle By Name(cluster=T12 {"paths"=[], "funnels"=[], "rects"=[], "dots"=[]} ("IDs"), "dots"=w1223, "funnels"=w1222, "rects"=w1221, "paths"=w1224) -> (w1220:T12)
        n440 = call "IDs to Names.vi"("IDs"=w1220) -> ("Names"=w1227:string[], "IDs"=w1219:string[])  [unwired: 9 in]
        n441 = call "Populate Registry.vi"("error in"=w1228, "Aliases"=w1227, "Names"=w1219) -> ("error out"=w1229:errorcluster)  [unwired: 8 in]
        n442 = call <vilib>:"Add State(s) to Queue__jki_lib_state_machine.vi"("State(s) in (\"\")"=w1232) -> ("States Out"=w1231:string)  [unwired: 14 in]
      }
      frame "---------- Parse ----------" {
        # "Parse: \n(Template Separater for Parsing. You can make a copy of, or modify, this frame)"
        n443 = Unbundle By Name(w1235) -> ("parser"=w1234:refnum<class "ParseVectorFile.lvclass">)
        n444 = Bundle By Name(cluster=w1235, "parser"=w1234) -> (w1236:T25)
        n445 = call <vilib>:"Add State(s) to Queue__jki_lib_state_machine.vi"("State(s) in (\"\")"=w1239) -> ("States Out"=w1238:string)  [unwired: 14 in]
      }
      frame "Parse: Send File" {
        # "Parse: \n(Template Separater for Parsing. You can make a copy of, or modify, this frame)"
        n446 = Unbundle By Name(w1247) -> ("parser"=w1245:refnum<class "ParseVectorFile.lvclass">, "UI.Inkscape File (.svg)"=w1243:path)
        n447 = call "ParseVectorFile.NewFileAsynchronous.vi"("error in (no error)"=w1241, "NewFile"=w1243, "ParseVectorFile"=w1245) -> ("error out"=w1242:errorcluster, "ParseVectorFile out"=w1244:refnum<class "ParseVectorFile.lvclass">)  [unwired: 7 in]
        n448 = Bundle By Name(cluster=w1247, "parser"=w1244) -> (w1248:T25)
        n449 = call <vilib>:"Add State(s) to Queue__jki_lib_state_machine.vi"("State(s) in (\"\")"=w1250) -> ("States Out"=w1249:string)  [unwired: 14 in]
      }
      frame "Parse: Stop" {
        # "Parse: \n(Template Separater for Parsing. You can make a copy of, or modify, this frame)"
        n450 = Unbundle By Name(w1259) -> ("parser"=w1254:refnum<class "ParseVectorFile.lvclass">)
        n451 = call <vilib>:"Stop.vi"("error in (no error)"=w1252, "SMO"=w1254) -> ("error out"=w1257:errorcluster, "SMO out"=w1256:refnum<class "ParseVectorFile.lvclass">)  [unwired: 8 in]
        n452 = call <vilib>:"Destroy.vi"("error in (no error)"=w1257, "SMO"=w1256) -> ("error out"=w1253:errorcluster)  [unwired: 9 in]
        n453 = Bundle By Name(cluster=w1259, "parser"=refnum<class "ParseVectorFile.lvclass"> refnum) -> (w1260:T25)
        n454 = call <vilib>:"Add State(s) to Queue__jki_lib_state_machine.vi"("State(s) in (\"\")"=w1262) -> ("States Out"=w1261:string)  [unwired: 14 in]
      }
      frame "Parse: Start" {
        # "Parse: \n(Template Separater for Parsing. You can make a copy of, or modify, this frame)"
        n455 = Unbundle By Name(w1271) -> ("parser"=w1267:refnum<class "ParseVectorFile.lvclass">)
        n456 = call <vilib>:"Create.vi"("error in (no error)"=w1264, "SMO"=w1267) -> ("error out"=w1268:errorcluster, "SMO out"=w1269:refnum<class "ParseVectorFile.lvclass">)  [unwired: 7 in, 1 out]
        n457 = call <vilib>:"Start.vi"("error in (no error)"=w1268, "SMO"=w1269) -> ("error out"=w1265:errorcluster, "SMO out"=w1266:refnum<class "ParseVectorFile.lvclass">)  [unwired: 8 in]
        n458 = Bundle By Name(cluster=w1271, "parser"=w1266) -> (w1272:T25)
        n459 = call <vilib>:"Add State(s) to Queue__jki_lib_state_machine.vi"("State(s) in (\"\")"=w1274) -> ("States Out"=w1273:string)  [unwired: 14 in]
      }
      frame "---------- Settings ----------" {
        # "Settings: \n(Template Separater for Settings. You can make a copy of, or modify, this frame)"
        n460 = Unbundle By Name(w1277) -> ("settings"=w1276:refnum<class "Setting Database.lvclass">)
        n461 = Bundle By Name(cluster=w1277, "settings"=w1276) -> (w1278:T25)
        n462 = call <vilib>:"Add State(s) to Queue__jki_lib_state_machine.vi"("State(s) in (\"\")"=w1281) -> ("States Out"=w1280:string)  [unwired: 14 in]
      }
      frame "Settings: Set Active" {
        # "Settings: \n(Template Separater for Settings. You can make a copy of, or modify, this frame)"
        n463 = Unbundle By Name(w1293) -> ("settings"=w1289:refnum<class "Setting Database.lvclass">)
        n464 = call "Query Registry.vi"("error in"=w1282, "Name In"=w1285) -> ("error out"=w1283:errorcluster, "Alias"=w1284:string)  [unwired: 6 in, 2 out]
        n465 = call "Name To Type.vi"("Name"=w1285) -> ("Type"=w1291:string)  [unwired: 4 in]
        n466 = call "Name To Index.vi"("Name"=w1285) -> ("Index"=w1290:i32)  [unwired: 4 in]
        n467 = case shown="\"f\"" w1291 {
          tunnel: w1289 -> [w1301 w1303 w1308 w1313 w1318 w1322]
          tunnel: [w1300 w1302 w1307 w1311 w1316 w1321] -> w1287
          tunnel: w1283 -> [w1297 w1302 w1306 w1310 w1315 w1320]
          tunnel: [w1301 w1303 w1305 w1312 w1317 w1323] -> w1288
          tunnel: w1290 -> [_ _ _ _ _ _]
          tunnel: w1284 -> [_ _ w1304 w1309 w1314 w1319]
          frame Default {
            n468 = call <vilib>:"Error Cluster From Error Code.vi"("error in (no error)"=w1297, "error message (\"\")"="Unknown Object Type. Cannot Set Active In Database" ("error message (\"\")"), "error code (0)"=1) -> ("error out"=w1300:errorcluster)  [unwired: 6 in]
          }
          frame "" {
            # "There are no objects to set as active\n\nTemp fix for issue \\#78:\nhttps://github.com/levylabpitt/AFM-Lithography/issues/78"
          }
          frame "p" {
            n469 = call "Setting Database.SetActivePath.vi"("error in (no error)"=w1306, "SetActivePath"=w1304, "Setting Database"=w1308) -> ("error out"=w1307:errorcluster, "Setting Database out"=w1305:refnum<class "Setting Database.lvclass">)  [unwired: 7 in]
          }
          frame "r" {
            n470 = call "Setting Database.SetActiveRectangle.vi"("error in (no error)"=w1310, "SetActiveRectangle"=w1309, "Setting Database"=w1313) -> ("error out"=w1311:errorcluster, "Setting Database out"=w1312:refnum<class "Setting Database.lvclass">)  [unwired: 7 in]
          }
          frame "f" {
            n471 = call "Setting Database.SetActiveFunnel.vi"("error in (no error)"=w1315, "SetActiveFunnel"=w1314, "Setting Database"=w1318) -> ("error out"=w1316:errorcluster, "Setting Database out"=w1317:refnum<class "Setting Database.lvclass">)  [unwired: 7 in]
          }
          frame "d" {
            # "Need to send the data event here"
            n472 = call "Setting Database.SetActiveDot.vi"("error in (no error)"=w1320, "SetActiveDot"=w1319, "Setting Database"=w1322) -> ("error out"=w1321:errorcluster, "Setting Database out"=w1323:refnum<class "Setting Database.lvclass">)  [unwired: 7 in]
          }
        }
        n473 = Bundle By Name(cluster=w1293, "settings"=w1288) -> (w1294:T25)
        n474 = call <vilib>:"Add State(s) to Queue__jki_lib_state_machine.vi"("State(s) in (\"\")"=w1296) -> ("States Out"=w1295:string)  [unwired: 14 in]
      }
      frame "Settings: Change Enable" {
        # "Settings: \n(Template Separater for Settings. You can make a copy of, or modify, this frame)"
        n475 = Unbundle By Name(w1331) -> ("settings"=w1329:refnum<class "Setting Database.lvclass">)
        n476 = call "Setting Database.ChangeObjectEnable.vi"("error in (no error)"=w1325, "ChangeObjectEnable"=w1327, "Setting Database"=w1329) -> ("error out"=w1326:errorcluster, "Setting Database out"=w1328:refnum<class "Setting Database.lvclass">)  [unwired: 7 in]
        n477 = Bundle By Name(cluster=w1331, "settings"=w1328) -> (w1332:T25)
        n478 = call <vilib>:"Add State(s) to Queue__jki_lib_state_machine.vi"("State(s) in (\"\")"=w1334) -> ("States Out"=w1333:string)  [unwired: 14 in]
      }
      frame "Settings: Group" {
        # "Settings: \n(Template Separater for Settings. You can make a copy of, or modify, this frame)"
        n479 = Unbundle By Name(w1349) -> ("settings"=w1347:refnum<class "Setting Database.lvclass">)
        n480 = Spreadsheet String To Array(delimiter (Tab)=":", format string="%s", spreadsheet string=w1344, array type (2D Dbl)=string[] []) -> (array=w1341:string[])
        n481 = Index Array(array=w1341) -> (element #1=w1338:string, element #2=w1340:string, element #3=w1339:string)  [unwired: 3 in]
        n482 = case shown="\"remove\"" w1338 {
          tunnel: w1347 -> [w1354 w1361 w1368 w1375]
          tunnel: [w1354 w1362 w1367 w1374] -> w1346
          tunnel: w1340 -> [_ w1359 w1370 w1371]
          tunnel: w1339 -> [_ w1358 w1369 _]
          tunnel: w1336 -> [w1353 w1356 w1366 w1373]
          tunnel: [w1353 w1355 w1365 w1372] -> w1337
          frame Default {
          }
          frame "add" {
            n483 = Bundle(cluster=T13 {"Name"="", "Group"=""} ("Add To Group"), "Name"=w1359, "Group"=w1358) -> (w1357:T13)
            n484 = call "Setting Database.AddToGroup.vi"("error in (no error)"=w1356, "Add To Group"=w1357, "Setting Database"=w1361) -> ("error out"=w1355:errorcluster, "Setting Database out"=w1362:refnum<class "Setting Database.lvclass">)  [unwired: 7 in]
          }
          frame "create" {
            n485 = Bundle(cluster=T14 {"Name"="", "Group"=""} ("Create New Group"), "Name"=w1370, "Group"=w1369) -> (w1363:T14)
            n486 = call "Setting Database.CreateNewGroup.vi"("error in (no error)"=w1366, "Create New Group"=w1363, "Setting Database"=w1368) -> ("error out"=w1365:errorcluster, "Setting Database out"=w1367:refnum<class "Setting Database.lvclass">)  [unwired: 7 in]
          }
          frame "remove" {
            n487 = call "Setting Database.RemoveFromGroup.vi"("error in (no error)"=w1373, "Remove From Group"=w1371, "Setting Database"=w1375) -> ("error out"=w1372:errorcluster, "Setting Database out"=w1374:refnum<class "Setting Database.lvclass">)  [unwired: 7 in]
          }
        }
        n488 = Bundle By Name(cluster=w1349, "settings"=w1346) -> (w1350:T25)
        n489 = call <vilib>:"Add State(s) to Queue__jki_lib_state_machine.vi"("State(s) in (\"\")"=w1352) -> ("States Out"=w1351:string)  [unwired: 14 in]
      }
      frame "Settings: Refresh" {
        # "Settings: \n(Template Separater for Settings. You can make a copy of, or modify, this frame)"
        n490 = Unbundle By Name(w1388) -> ("settings"=w1386:refnum<class "Setting Database.lvclass">, "GUIDs.Paths"=w1384:string[], "GUIDs.Rects"=w1382:string[], "GUIDs.Funnels"=w1381:string[], "GUIDs.Dots"=w1380:string[])
        n491 = Bundle By Name(cluster=T15 {"Paths"=[], "Rectangles"=[], "Funnels"=[], "Dots"=[]} ("Initialize"), "Paths"=w1384, "Rectangles"=w1382, "Funnels"=w1381, "Dots"=w1380) -> (w1379:T15)
        n492 = call "Setting Database.Refresh.vi"("error in (no error)"=w1378, "Initialize"=w1379, "Setting Database"=w1386) -> ("error out"=w1377:errorcluster, "Setting Database out"=w1385:refnum<class "Setting Database.lvclass">)  [unwired: 7 in]
        n493 = Bundle By Name(cluster=w1388, "settings"=w1385) -> (w1389:T25)
        n494 = call <vilib>:"Add State(s) to Queue__jki_lib_state_machine.vi"("State(s) in (\"\")"=w1391) -> ("States Out"=w1390:string)  [unwired: 14 in]
      }
      frame "Settings: Stop" {
        # "Settings: \n(Template Separater for Settings. You can make a copy of, or modify, this frame)"
        n495 = Unbundle By Name(w1400) -> ("settings"=w1397:refnum<class "Setting Database.lvclass">)
        n496 = call <vilib>:"Stop.vi"("error in (no error)"=w1394, "SMO"=w1397) -> ("error out"=w1398:errorcluster, "SMO out"=w1396:refnum<class "Setting Database.lvclass">)  [unwired: 8 in]
        n497 = call <vilib>:"Destroy.vi"("error in (no error)"=w1398, "SMO"=w1396) -> ("error out"=w1393:errorcluster)  [unwired: 9 in]
        n498 = Bundle By Name(cluster=w1400, "settings"=refnum<class "Setting Database.lvclass"> refnum) -> (w1401:T25)
        n499 = call <vilib>:"Add State(s) to Queue__jki_lib_state_machine.vi"("State(s) in (\"\")"=w1403) -> ("States Out"=w1402:string)  [unwired: 14 in]
      }
      frame "Settings: Start" {
        # "Settings: \n(Template Separater for Settings. You can make a copy of, or modify, this frame)"
        n500 = Unbundle By Name(w1415) -> ("settings"=w1410:refnum<class "Setting Database.lvclass">)
        n501 = call "Setting Database Name.vi"("error in (no error)"=w1406) -> ("error out"=w1407:errorcluster, "Name"=w1405:string)  [unwired: 9 in]
        n502 = call <vilib>:"Create.vi"("Shared Resource (F)"=TRUE, "error in (no error)"=w1407, "Subsystem Name (optional)"=w1405, "SMO"=w1410) -> ("error out"=w1412:errorcluster, "SMO out"=w1413:refnum<class "Setting Database.lvclass">)  [unwired: 5 in, 1 out]
        n503 = call <vilib>:"Start.vi"("error in (no error)"=w1412, "SMO"=w1413) -> ("error out"=w1409:errorcluster, "SMO out"=w1411:refnum<class "Setting Database.lvclass">)  [unwired: 8 in]
        n504 = Bundle By Name(cluster=w1415, "settings"=w1411) -> (w1416:T25)
        n505 = call <vilib>:"Add State(s) to Queue__jki_lib_state_machine.vi"("State(s) in (\"\")"=w1418) -> ("States Out"=w1417:string)  [unwired: 14 in]
      }
      frame "---------- Tool ----------" {
        # "Tool: \n(Template Separater for Tooling. You can make a copy of, or modify, this frame)"
        n506 = Unbundle By Name(w1421) -> ("tooler"=w1420:refnum<class "Tool Data.lvclass">)
        n507 = Bundle By Name(cluster=w1421, "tooler"=w1420) -> (w1422:T25)
        n508 = call <vilib>:"Add State(s) to Queue__jki_lib_state_machine.vi"("State(s) in (\"\")"=w1425) -> ("States Out"=w1424:string)  [unwired: 14 in]
      }
      frame "Tool: Sort Paths" {
        # "Tool: \n(Template Separater for Tooling. You can make a copy of, or modify, this frame)"
        n509 = Unbundle By Name(w1440) -> ("Parsed Obj.Paths"=w1431:refnum<class "Path.lvclass">[])
        n510 = call-dynamic "Write Paths Data.vi"("error in (no error)"=w1427, "Paths"=w1431, "Tool Data in"=refnum<class "Tool Data.lvclass"> refnum) -> ("error out"=w1436:errorcluster, "Tool Data out"=w1433:refnum<class "Tool Data.lvclass">)  [unwired: 7 in]
        n511 = call "Sort Funnels and Paths.vi"("error in (no error)"=w1436, "Tool Data in"=w1433) -> ("error out"=w1437:errorcluster, "Tool Data out"=w1434:refnum<class "Tool Data.lvclass">)  [unwired: 8 in]
        n512 = call-dynamic "Read Paths Data.vi"("error in (no error)"=w1437, "Tool Data in"=w1434) -> ("error out"=w1438:errorcluster, "Paths"=w1430:refnum<class "Path.lvclass">[], "Tool Data out"=w1435:refnum<class "Tool Data.lvclass">)  [unwired: 7 in]
        n513 = call-dynamic "Read Funnels Data.vi"("error in (no error)"=w1438, "Tool Data in"=w1435) -> ("error out"=w1428:errorcluster, "Funnels"=w1429:refnum<class "Path.lvclass">[])  [unwired: 7 in, 1 out]
        n514 = Bundle By Name(cluster=w1440, "Parsed Obj.Paths"=w1430, "Parsed Obj.Funnels"=w1429) -> (w1441:T25)
        n515 = call <vilib>:"Add State(s) to Queue__jki_lib_state_machine.vi"("State(s) in (\"\")"=w1443) -> ("States Out"=w1442:string)  [unwired: 14 in]
      }
      frame "Tool: Get IDs" {
        # "Tool: \n(Template Separater for Tooling. You can make a copy of, or modify, this frame)"
        n516 = Unbundle By Name(w1457) -> ("Parsed Obj.Paths"=w1448:refnum<class "Path.lvclass">[], "Parsed Obj.Rectangles"=w1444:refnum<class "Rectangle.lvclass">[], "Parsed Obj.Background"=w1445:refnum<class "SVGImage.lvclass">, "Parsed Obj.Dots"=w1446:refnum<class "Dot.lvclass">[], "Parsed Obj.Funnels"=w1447:refnum<class "Path.lvclass">[])
        n517 = Bundle By Name(cluster=T16 {"Paths"=[], "Rectangles"=[], "SVGImage"=refnum, "Dots"=[], "Funnels"=[]} ("Data"), "Paths"=w1448, "Rectangles"=w1444, "SVGImage"=w1445, "Dots"=w1446, "Funnels"=w1447) -> (w1449:T16)
        n518 = property class="Tool Data.lvclass"(reference=refnum<class "Tool Data.lvclass"> refnum ("Tool Data in"), error in=w1458, "Accessors:Data"=w1449) -> (reference out=w1461:refnum<class "Tool Data.lvclass">, error out=w1459:errorcluster)
        n519 = call "Get IDs.vi"("error in (no error)"=w1459, "Tool Data in"=w1461) -> ("error out"=w1462:errorcluster, "IDs"=w1455:T12)  [unwired: 7 in, 1 out]
        n520 = Unbundle By Name(w1455) -> ("paths"=w1454:string[], "funnels"=w1453:string[], "rects"=w1452:string[], "dots"=w1451:string[])
        n521 = Bundle By Name(cluster=w1457, "GUIDs.Paths"=w1454, "GUIDs.Funnels"=w1453, "GUIDs.Rects"=w1452, "GUIDs.Dots"=w1451) -> (w1464:T25)
        n522 = call <vilib>:"Add State(s) to Queue__jki_lib_state_machine.vi"("State(s) in (\"\")"=w1466) -> ("States Out"=w1465:string)  [unwired: 14 in]
      }
      frame "Tool: Generate Litho Data" {
        # "Tool: \n(Template Separater for Tooling. You can make a copy of, or modify, this frame)"
        n523 = Unbundle By Name(w1477) -> ("tooler"=w1475:refnum<class "Tool Data.lvclass">)
        n524 = call-dynamic "Generate Lithography Data.vi"("error in (no error)"=w1472, "Tool Data in"=w1475) -> ("error out"=w1473:errorcluster, "Lithography Data"=w1468:T30, "Tool Data out"=w1474:refnum<class "Tool Data.lvclass">)  [unwired: 7 in]
        n525 = call "Estimated Time Required.vi"("Lithography Data"=w1468) -> ("Estimated Time Required"=w1470:timestamp)
        n526 = Bundle By Name(cluster=w1477, "tooler"=w1474, "Litho"=w1468) -> (w1478:T25)
        n527 = Format Date/Time String(time format string (%c)="UI: Update Control >> Estimated Time >> %H:%M:%S", seconds (now)=w1470) -> (date/time string=w1467:string)  [unwired: 1 in]
        n528 = call <vilib>:"Add State(s) to Queue__jki_lib_state_machine.vi"("State(s) in Front (\"\")"=w1467, "State(s) in (\"\")"=w1480) -> ("States Out"=w1479:string)  [unwired: 13 in]
      }
      frame "Tool: Objects" {
        # "Tool: \n(Template Separater for Tooling. You can make a copy of, or modify, this frame)"
        n529 = Unbundle By Name(w1500) -> ("tooler"=w1491:refnum<class "Tool Data.lvclass">, "Parsed Obj.Paths"=w1482:refnum<class "Path.lvclass">[], "Parsed Obj.Funnels"=w1481:refnum<class "Path.lvclass">[], "Parsed Obj.Rectangles"=w1497:refnum<class "Rectangle.lvclass">[], "Parsed Obj.Dots"=w1496:refnum<class "Dot.lvclass">[], "Obj Settings.Paths"=w1495:T18, "Obj Settings.Rectangles"=w1494:T19, "Obj Settings.Funnels"=w1493:T20, "Obj Settings.Dots"=w1492:T21)
        n530 = Bundle By Name(cluster=T17 {"Settings"={"Paths"=[], "Rectangles"=[], "Funnels"=[], "Dots"=[]}, "Data"={"Paths"=[], "Rectangles"=[], "SVGImage"=refnum, "Dots"=[], "Funnels"=[]}} ("Updated Objects"), "Data.Paths"=w1482, "Data.Funnels"=w1481, "Data.Rectangles"=w1497, "Data.Dots"=w1496, "Settings.Paths"=w1495, "Settings.Rectangles"=w1494, "Settings.Funnels"=w1493, "Settings.Dots"=w1492) -> (w1490:T17)
        n531 = call "Tool Data.UpdateObjects.vi"("error in (no error)"=w1486, "Updated Objects"=w1490, "Tool Data"=w1491) -> ("error out"=w1488:errorcluster, "Tool Data out"=w1485:refnum<class "Tool Data.lvclass">)  [unwired: 7 in]
        n532 = call-dynamic "Find Changed.vi"("error in (no error)"=w1488, "Update Objects"=w1490, "Tool Data in"=w1485) -> ("error out"=w1487:errorcluster, "Changed Objects"=w1489:T33, "Tool Data out"=w1484:refnum<class "Tool Data.lvclass">)  [unwired: 6 in]
        n533 = Bundle By Name(cluster=w1500, "tooler"=w1484, "Changed Obj"=w1489) -> (w1501:T25)
        n534 = call <vilib>:"Add State(s) to Queue__jki_lib_state_machine.vi"("State(s) in (\"\")"=w1503) -> ("States Out"=w1502:string)  [unwired: 14 in]
      }
      frame "Tool: Stop" {
        # "Tool: \n(Template Separater for Tooling. You can make a copy of, or modify, this frame)"
        n535 = Unbundle By Name(w1513) -> ("tooler"=w1509:refnum<class "Tool Data.lvclass">)
        n536 = call <vilib>:"Stop.vi"("timeout in ms (-1)"=10000, "error in (no error)"=w1507, "SMO"=w1509) -> ("error out"=w1511:errorcluster, "SMO out"=w1510:refnum<class "Tool Data.lvclass">)  [unwired: 7 in]
        n537 = call <vilib>:"Destroy.vi"("error in (no error)"=w1511, "SMO"=w1510) -> ("error out"=w1508:errorcluster)  [unwired: 9 in]
        n538 = Bundle By Name(cluster=w1513, "tooler"=refnum<class "Tool Data.lvclass"> refnum) -> (w1514:T25)
        n539 = call <vilib>:"Add State(s) to Queue__jki_lib_state_machine.vi"("State(s) in (\"\")"=w1516) -> ("States Out"=w1515:string)  [unwired: 14 in]
      }
      frame "Tool: Start" {
        # "Tool: \n(Template Separater for Tooling. You can make a copy of, or modify, this frame)"
        n540 = Unbundle By Name(w1525) -> ("tooler"=w1521:refnum<class "Tool Data.lvclass">)
        n541 = call <vilib>:"Create.vi"("error in (no error)"=w1518, "SMO"=w1521) -> ("error out"=w1522:errorcluster, "SMO out"=w1523:refnum<class "Tool Data.lvclass">)  [unwired: 7 in, 1 out]
        n542 = call <vilib>:"Start.vi"("error in (no error)"=w1522, "SMO"=w1523) -> ("error out"=w1519:errorcluster, "SMO out"=w1520:refnum<class "Tool Data.lvclass">)  [unwired: 8 in]
        n543 = Bundle By Name(cluster=w1525, "tooler"=w1520) -> (w1526:T25)
        n544 = call <vilib>:"Add State(s) to Queue__jki_lib_state_machine.vi"("State(s) in (\"\")"=w1528) -> ("States Out"=w1527:string)  [unwired: 14 in]
      }
      frame "---------- Big MAQ ----------" {
        # "Parse: \n(Template Separater for Parsing. You can make a copy of, or modify, this frame)"
        n545 = Unbundle By Name(w1531) -> ("big-maq"=w1530:refnum<class "BigMAQ.lvclass">)
        n546 = Bundle By Name(cluster=w1531, "big-maq"=w1530) -> (w1532:T25)
        n547 = call <vilib>:"Add State(s) to Queue__jki_lib_state_machine.vi"("State(s) in (\"\")"=w1535) -> ("States Out"=w1534:string)  [unwired: 14 in]
      }
      frame "Big MAQ: Coerce Size" {
        # "Parse: \n(Template Separater for Parsing. You can make a copy of, or modify, this frame)"
        n548 = Unbundle By Name(w1553) -> ("big-maq"=w1540:refnum<class "BigMAQ.lvclass">, "Parsed Obj.Background"=w1551:refnum<class "SVGImage.lvclass">)
        n549 = call "Read Height.vi"("error in (no error)"=w1548, "Image in"=w1551) -> ("error out"=w1538:errorcluster, "Height"=w1550:dbl)  [unwired: 7 in, 1 out]
        n550 = Divide(x=w1550, y=1000.0) -> (x/y=w1545:dbl)
        n551 = call-dynamic "Read ScanSize.vi"("error in (no error)"=w1538, "BigMAQ in"=w1540) -> ("error out"=w1537:errorcluster, "ScanSize"=w1536:dbl, "BigMAQ out"=w1539:refnum<class "BigMAQ.lvclass">)  [unwired: 7 in]
        n552 = Equal?(x=w1536, y=w1545) -> (x = y?=w1541:bool)
        n553 = case shown="False" w1541 {
          tunnel: w1539 -> [w1561 w1563]
          tunnel: [w1560 w1563] -> w1547
          tunnel: w1537 -> [w1559 w1562]
          tunnel: [w1558 w1562] -> w1546
          tunnel: w1545 -> [w1557 _]
          frame False {
            n554 = call-dynamic "Write Size.vi"("error in (no error)"=w1559, "Size"=w1557, "BigMAQ in"=w1561) -> ("error out"=w1558:errorcluster, "BigMAQ out"=w1560:refnum<class "BigMAQ.lvclass">)  [unwired: 7 in]
          }
          frame True {
          }
        }
        n555 = local write "Sizes Match?"(w1541) -> ()
        n556 = Bundle By Name(cluster=w1553, "big-maq"=w1547) -> (w1554:T25)
        n557 = Select(t="", s=w1541, f="AFM image and Inkscape file image do not  match. ::Using Inkscape file size::") -> (s? t:f=w1542:string)
        n558 = call <vilib>:"Add State(s) to Queue__jki_lib_state_machine.vi"("State(s) in (\"\")"=w1556) -> ("States Out"=w1555:string)  [unwired: 14 in]
      }
      frame "Big MAQ: Labels" {
        # "Parse: \n(Template Separater for Parsing. You can make a copy of, or modify, this frame)"
        n559 = Unbundle By Name(w1576) -> ("big-maq"=w1571:refnum<class "BigMAQ.lvclass">, "Litho"=w1566:T30)
        n560 = To Upper Case(1:w1572) -> (0:w1564:string)
        n561 = Match True/False String(2:"SHOW" ("false string"), 3:"HIDE" ("true string"), 4:w1564) -> (0:w1567:bool)  [unwired: 1 out]
        n562 = call "Label Visibility.vi"("Show Text"=w1567, "error in"=w1568, "Lithography Data"=w1566, "BigMAQ in"=w1571) -> ("error out"=w1569:errorcluster, "BigMAQ out"=w1570:refnum<class "BigMAQ.lvclass">)  [unwired: 6 in]
        n563 = Bundle By Name(cluster=w1576, "big-maq"=w1570) -> (w1577:T25)
        n564 = call <vilib>:"Add State(s) to Queue__jki_lib_state_machine.vi"("State(s) in (\"\")"=w1579) -> ("States Out"=w1578:string)  [unwired: 14 in]
      }
      frame "Big MAQ: Zoom Fit" {
        # "Parse: \n(Template Separater for Parsing. You can make a copy of, or modify, this frame)"
        n565 = Unbundle By Name(w1588) -> ("big-maq"=w1587:refnum<class "BigMAQ.lvclass">)
        n566 = call "Zoom to Fit.vi"("error in"=w1584, "BigMAQ in"=w1587) -> ("error out"=w1585:errorcluster, "ZoomSingle"=w1581:cluster{"X":sgl, "Y":sgl}, "BigMAQ out"=w1586:refnum<class "BigMAQ.lvclass">)  [unwired: 7 in]
        n567 = Build Array(w1581) -> (w1580:cluster{"X":sgl, "Y":sgl}[])
        n568 = Bundle By Name(cluster=w1588, "big-maq"=w1586, "Zoom History"=w1580) -> (w1589:T25)
        n569 = call <vilib>:"Add State(s) to Queue__jki_lib_state_machine.vi"("State(s) in (\"\")"=w1591) -> ("States Out"=w1590:string)  [unwired: 14 in]
      }
      frame "Big MAQ: Update" {
        # "Parse: \n(Template Separater for Parsing. You can make a copy of, or modify, this frame)"
        n570 = Unbundle By Name(w1598) -> ("big-maq"=w1597:refnum<class "BigMAQ.lvclass">)
        n571 = call "Update Control.vi"("error in"=w1594, "BigMAQ in"=w1597) -> ("error out"=w1595:errorcluster, "BigMAQ out"=w1596:refnum<class "BigMAQ.lvclass">)  [unwired: 8 in]
        n572 = Bundle By Name(cluster=w1598, "big-maq"=w1596) -> (w1599:T25)
        n573 = call <vilib>:"Add State(s) to Queue__jki_lib_state_machine.vi"("State(s) in (\"\")"=w1601) -> ("States Out"=w1600:string)  [unwired: 14 in]
      }
      frame "Big MAQ: Generate Overlay" {
        # "Parse: \n(Template Separater for Parsing. You can make a copy of, or modify, this frame)"
        n574 = Unbundle By Name(w1612) -> ("big-maq"=w1611:refnum<class "BigMAQ.lvclass">, "Litho"=w1603:T30, "UI.Hide Labels"=w1607:bool, "UI.Pixellate?"=w1602:bool)
        n575 = Not(x=w1607) -> (.not. x?=w1606:bool)
        n576 = call "Generate New Overlay.vi"("Pixellate"=w1602, "Label?"=w1606, "error in"=w1608, "Lithography Data"=w1603, "BigMAQ in"=w1611) -> ("error out"=w1609:errorcluster, "BigMAQ out"=w1610:refnum<class "BigMAQ.lvclass">)  [unwired: 5 in]
        n577 = Bundle By Name(cluster=w1612, "big-maq"=w1610) -> (w1613:T25)
        n578 = call <vilib>:"Add State(s) to Queue__jki_lib_state_machine.vi"("State(s) in (\"\")"=w1615) -> ("States Out"=w1614:string)  [unwired: 14 in]
      }
      frame "Big MAQ: Select Page" {
        # "Update the page control"
        # "Parse: \n(Template Separater for Parsing. You can make a copy of, or modify, this frame)"
        n579 = Unbundle By Name(w1628) -> ("big-maq"=w1627:refnum<class "BigMAQ.lvclass">, "UI.Page"=w1625:u32)
        n580 = call "Select Page.vi"("error in (no error)"=w1619, "Page"=w1625, "BigMAQ in"=w1627) -> ("error out"=w1620:errorcluster, "Corrected Page"=w1624:u32, "BigMAQ out"=w1626:refnum<class "BigMAQ.lvclass">)  [unwired: 6 in]
        n581 = Equal?(x=w1624, y=w1625) -> (x = y?=w1623:bool)
        n582 = Bundle By Name(cluster=w1628, "big-maq"=w1626) -> (w1629:T25)
        n583 = Select(t="", s=w1623, f="UI: Update Control >> Page") -> (s? t:f=w1622:string)
        n584 = call <vilib>:"Add State(s) to Queue__jki_lib_state_machine.vi"("State(s) in Front (\"\")"=w1622, "State(s) in (\"\")"=w1631) -> ("States Out"=w1630:string)  [unwired: 13 in]
      }
      frame "Big MAQ: Change Data Range" {
        # "Parse: \n(Template Separater for Parsing. You can make a copy of, or modify, this frame)"
        n585 = Unbundle By Name(w1643) -> ("big-maq"=w1642:refnum<class "BigMAQ.lvclass">, "UI.Image Data Range"=w1638:cluster{sgl, sgl})
        n586 = Unbundle(w1638) -> (w1637:sgl, w1636:sgl)
        n587 = Max & Min(x=w1637, y=w1636) -> (max(x,y)=w1635:sgl, min(x,y)=w1634:sgl)
        n588 = call "Change Data Range.vi"("error in"=w1639, "Minimum"=w1634, "Maximum"=w1635, "BigMAQ in"=w1642) -> ("error out"=w1640:errorcluster, "BigMAQ out"=w1641:refnum<class "BigMAQ.lvclass">)  [unwired: 6 in]
        n589 = Bundle By Name(cluster=w1643, "big-maq"=w1641) -> (w1644:T25)
        n590 = call <vilib>:"Add State(s) to Queue__jki_lib_state_machine.vi"("State(s) in (\"\")"=w1646) -> ("States Out"=w1645:string)  [unwired: 14 in]
      }
      frame "Big MAQ: Read Background" {
        # "Parse: \n(Template Separater for Parsing. You can make a copy of, or modify, this frame)"
        n591 = Unbundle By Name(w1656) -> ("big-maq"=w1655:refnum<class "BigMAQ.lvclass">, "UI.Background Image"=w1653:path)
        n592 = call "Read Background.vi"("error in (no error)"=w1651, "Path"=w1653, "BigMAQ in"=w1655) -> ("error out"=w1652:errorcluster, "BigMAQ out"=w1654:refnum<class "BigMAQ.lvclass">)  [unwired: 6 in, 1 out]
        n593 = Bundle By Name(cluster=w1656, "big-maq"=w1654, "UI.Page"=u32 0) -> (w1657:T25)
        n594 = call <vilib>:"Add State(s) to Queue__jki_lib_state_machine.vi"("State(s) in Front (\"\")"="UI: Update Control >> Page\nBig MAQ: Save Background", "State(s) in (\"\")"=w1659) -> ("States Out"=w1658:string)  [unwired: 13 in]
      }
      frame "Big MAQ: Save Background" {
        # "Parse: \n(Template Separater for Parsing. You can make a copy of, or modify, this frame)"
        n595 = Unbundle By Name(w1668) -> ("big-maq"=w1666:refnum<class "BigMAQ.lvclass">, "UI.Inkscape File (.svg)"=w1662:path)
        n596 = call "Get Background Image JPG Path.vi"("Inkscape Path"=w1662) -> ("Background JPG Path"=w1661:path)  [unwired: 2 in]
        n597 = call "Save Background.vi"("error in"=w1660, "File Path"=w1661, "BigMAQ in"=w1666) -> ("error out"=w1664:errorcluster, "BigMAQ out"=w1665:refnum<class "BigMAQ.lvclass">)  [unwired: 7 in]
        n598 = Bundle By Name(cluster=w1668, "big-maq"=w1665) -> (w1669:T25)
        n599 = call <vilib>:"Add State(s) to Queue__jki_lib_state_machine.vi"("State(s) in (\"\")"=w1671) -> ("States Out"=w1670:string)  [unwired: 14 in]
      }
      frame "Big MAQ: Save Render" {
        # "Parse: \n(Template Separater for Parsing. You can make a copy of, or modify, this frame)"
        n600 = Unbundle By Name(w1680) -> ("big-maq"=w1679:refnum<class "BigMAQ.lvclass">, "UI.Normal Save Path"=w1673:path)
        n601 = call "Save Image to Disk.vi"("Image Quality"=u32 1024, "error in"=w1676, "Path"=w1673, "BigMAQ in"=w1679) -> ("error out"=w1677:errorcluster, "BigMAQ out"=w1678:refnum<class "BigMAQ.lvclass">)  [unwired: 6 in]
        n602 = Bundle By Name(cluster=w1680, "big-maq"=w1678) -> (w1681:T25)
        n603 = call <vilib>:"Add State(s) to Queue__jki_lib_state_machine.vi"("State(s) in (\"\")"=w1683) -> ("States Out"=w1682:string)  [unwired: 14 in]
      }
      frame "Big MAQ: Copy Render" {
        # "Parse: \n(Template Separater for Parsing. You can make a copy of, or modify, this frame)"
        n604 = Unbundle By Name(w1690) -> ("big-maq"=w1687:refnum<class "BigMAQ.lvclass">)
        n605 = call "Copy Render to Clipboard.vi"("error in"=w1685, "BigMAQ in"=w1687) -> ("error out"=w1684:errorcluster, "BigMAQ out"=w1686:refnum<class "BigMAQ.lvclass">)  [unwired: 8 in]
        n606 = Bundle By Name(cluster=w1690, "big-maq"=w1686) -> (w1691:T25)
        n607 = call <vilib>:"Add State(s) to Queue__jki_lib_state_machine.vi"("State(s) in (\"\")"=w1693) -> ("States Out"=w1692:string)  [unwired: 14 in]
      }
      frame "Big MAQ: Autosave Render" {
        # "Need to change the path to align with the overwrite control"
        # "Parse: \n(Template Separater for Parsing. You can make a copy of, or modify, this frame)"
        n608 = Unbundle By Name(w1710) -> ("big-maq"=w1709:refnum<class "BigMAQ.lvclass">, "UI.Autosave Path"=w1697:path, "UI.Autosave?"=w1702:bool, "UI.Overwrite"=w1695:bool)
        n609 = Strip Path(path=w1697) -> (stripped path=w1699:path)  [unwired: 1 out]
        n610 = Format Date/Time String(time format string (%c)="%d_%m_%Y-%H_%M_%S.jpg") -> (date/time string=w1694:string)  [unwired: 2 in]
        n611 = Build Path(base path=w1699, name or relative path=w1694) -> (appended path=w1698:path)
        n612 = Select(t=w1697, s=w1695, f=w1698) -> (s? t:f=w1696:path)
        n613 = case shown="True" w1702 {
          tunnel: w1709 -> [w1714 w1721]
          tunnel: [w1714 w1720] -> w1708
          tunnel: [w1715 w1719] -> w1707
          tunnel: w1706 -> [w1715 w1718]
          tunnel: w1696 -> [_ w1717]
          frame False {
          }
          frame True {
            n614 = call "Save Image to Disk.vi"("Image Quality"=u32 512, "error in"=w1718, "Path"=w1717, "BigMAQ in"=w1721) -> ("error out"=w1719:errorcluster, "BigMAQ out"=w1720:refnum<class "BigMAQ.lvclass">)  [unwired: 6 in]
          }
        }
        n615 = Bundle By Name(cluster=w1710, "big-maq"=w1708) -> (w1711:T25)
        n616 = Select(t="Render Autosaved to Disk", s=w1702, f="") -> (s? t:f=w1701:string)
        n617 = call <vilib>:"Add State(s) to Queue__jki_lib_state_machine.vi"("State(s) in (\"\")"=w1713) -> ("States Out"=w1712:string)  [unwired: 14 in]
      }
      frame "Big MAQ: Cleanup" {
        # "Parse: \n(Template Separater for Parsing. You can make a copy of, or modify, this frame)"
        n618 = Unbundle By Name(w1728) -> ("big-maq"=w1727:refnum<class "BigMAQ.lvclass">)
        n619 = call <vilib>:"Destroy.vi"("error in"=w1724, "BigMAQ in"=w1727) -> ("error out"=w1725:errorcluster, "BigMAQ out"=w1726:refnum<class "BigMAQ.lvclass">)  [unwired: 8 in]
        n620 = Bundle By Name(cluster=w1728, "big-maq"=w1726) -> (w1729:T25)
        n621 = call <vilib>:"Add State(s) to Queue__jki_lib_state_machine.vi"("State(s) in (\"\")"=w1731) -> ("States Out"=w1730:string)  [unwired: 14 in]
      }
      frame "Big MAQ: Initialize" {
        # "Parse: \n(Template Separater for Parsing. You can make a copy of, or modify, this frame)"
        n622 = control-ref of="Render"() -> (w1738:refnum<vi>)
        n623 = call <vilib>:"Create.vi"("error in (no error)"=w1741, "Resolution"=1024, "Reference"=w1738) -> ("error out"=w1734:errorcluster, "To Control"=→"Render":T2, "BigMAQ out"=w1737:refnum<class "BigMAQ.lvclass">)  [unwired: 6 in]
        n624 = call-dynamic "Write Voltage Scale.vi"("error in (no error)"=w1734, "Voltage Scale"=20.0, "BigMAQ in"=w1737) -> ("error out"=w1733:errorcluster, "BigMAQ out"=w1736:refnum<class "BigMAQ.lvclass">)  [unwired: 7 in]
        n625 = Bundle By Name(cluster=w1743, "big-maq"=w1736) -> (w1744:T25)
        n626 = call <vilib>:"Add State(s) to Queue__jki_lib_state_machine.vi"("State(s) in (\"\")"=w1746) -> ("States Out"=w1745:string)  [unwired: 14 in]
      }
      frame "---------- Select ----------" {
        # "Select: \n(Template Separater for Selector i.e. MCLB. You can make a copy of, or modify, this frame)"
        n627 = Unbundle By Name(w1749) -> ("selector"=w1748:refnum<class "Selector.lvclass">)
        n628 = Bundle By Name(cluster=w1749, "selector"=w1748) -> (w1750:T25)
        n629 = call <vilib>:"Add State(s) to Queue__jki_lib_state_machine.vi"("State(s) in (\"\")"=w1753) -> ("States Out"=w1752:string)  [unwired: 14 in]
      }
      frame "Select: Change By Name" {
        # "Select: \n(Template Separater for Selector i.e. MCLB. You can make a copy of, or modify, this frame)"
        n630 = Unbundle By Name(w1755) -> ("GUIDs"=w1757:T32)
        n631 = case shown="\"first\"" w1754 {
          selector: w1754 -> [w1771 _]
          tunnel: [w1771 w1772] -> w1758
          tunnel: w1757 -> [_ w1780]
          frame Default {
          }
          frame "first" {
            n632 = Unbundle(w1780) -> ("Dots"=w1775:string[], "Funnels"=w1776:string[], "Rects"=w1777:string[], "Paths"=w1778:string[])
            n633 = Bundle(cluster=T12 {"paths"=[], "funnels"=[], "rects"=[], "dots"=[]} ("IDs"), "paths"=w1778, "funnels"=w1776, "rects"=w1777, "dots"=w1775) -> (w1774:T12)
            n634 = call "IDs to Names.vi"("IDs"=w1774) -> ("Names"=w1773:string[])  [unwired: 9 in, 1 out]
            n635 = Index Array(array=w1773) -> (element=w1772:string)  [unwired: 1 in]
          }
        }
        n636 = Unbundle By Name(w1755) -> ("selector"=w1763:refnum<class "Selector.lvclass">)
        n637 = call "Model--Set Value by Name.vi"("error in"=w1760, "Name"=w1758, "Selector in"=w1763) -> ("error out"=w1761:errorcluster, "element"=w1759:T41, "Selector out"=w1762:refnum<class "Selector.lvclass">)  [unwired: 6 in]
        n638 = Unbundle By Name(w1759) -> ("Name"=w1766:string)
        n639 = Bundle By Name(cluster=w1755, "selector"=w1762) -> (w1768:T25)
        n640 = call <vilib>:"Build State String with Arguments__JKI_lib_State_Machine.vi"("Arguments (\"\")"=w1766, "State"="Subpanel: Insert") -> ("State with Arguments"=w1764:string)  [unwired: 4 in]
        n641 = call <vilib>:"Add State(s) to Queue__jki_lib_state_machine.vi"("State(s) in Front (\"\")"=w1764, "State(s) in (\"\")"=w1770) -> ("States Out"=w1769:string)  [unwired: 13 in]
      }
      frame "Select: New Name Set" {
        # "Select: \n(Template Separater for Selector i.e. MCLB. You can make a copy of, or modify, this frame)"
        n642 = Unbundle By Name(w1795) -> ("selector"=w1793:refnum<class "Selector.lvclass">, "GUIDs"=w1783:T32)
        n643 = Unbundle By Name(w1783) -> ("Paths"=w1787:string[], "Funnels"=w1784:string[], "Rects"=w1785:string[], "Dots"=w1786:string[])
        n644 = Bundle By Name(cluster=T12 {"paths"=[], "funnels"=[], "rects"=[], "dots"=[]} ("IDs"), "paths"=w1787, "funnels"=w1784, "rects"=w1785, "dots"=w1786) -> (w1782:T12)
        n645 = call "IDs to Names.vi"("IDs"=w1782) -> ("Names"=w1791:string[])  [unwired: 9 in, 1 out]
        n646 = call-dynamic "Compare New Values.vi"("error in (no error)"=w1789, "New Values"=w1791, "Selector in"=w1793) -> ("error out"=w1790:errorcluster, "Selector out"=w1792:refnum<class "Selector.lvclass">)  [unwired: 6 in, 1 out]
        n647 = Bundle By Name(cluster=w1795, "selector"=w1792) -> (w1796:T25)
        n648 = call <vilib>:"Add State(s) to Queue__jki_lib_state_machine.vi"("State(s) in (\"\")"=w1798) -> ("States Out"=w1797:string)  [unwired: 14 in]
      }
      frame "Select: Update" {
        # "Select: \n(Template Separater for Selector i.e. MCLB. You can make a copy of, or modify, this frame)"
        n649 = Unbundle By Name(w1805) -> ("selector"=w1803:refnum<class "Selector.lvclass">)
        n650 = call "UI--Update.vi"("error in"=w1800, "Selector in"=w1803) -> ("error out"=w1801:errorcluster, "Selector out"=w1802:refnum<class "Selector.lvclass">)  [unwired: 8 in]
        n651 = Bundle By Name(cluster=w1805, "selector"=w1802) -> (w1806:T25)
        n652 = call <vilib>:"Add State(s) to Queue__jki_lib_state_machine.vi"("State(s) in (\"\")"=w1808) -> ("States Out"=w1807:string)  [unwired: 14 in]
      }
      frame "Select: Apply Symbols" {
        # "Select: \n(Template Separater for Selector i.e. MCLB. You can make a copy of, or modify, this frame)"
        n653 = Unbundle By Name(w1815) -> ("selector"=w1813:refnum<class "Selector.lvclass">)
        n654 = call "UI--Apply Item Symbols.vi"("error in"=w1810, "Selector in"=w1813) -> ("error out"=w1811:errorcluster, "Selector out"=w1812:refnum<class "Selector.lvclass">)  [unwired: 8 in]
        n655 = Bundle By Name(cluster=w1815, "selector"=w1812) -> (w1816:T25)
        n656 = call <vilib>:"Add State(s) to Queue__jki_lib_state_machine.vi"("State(s) in (\"\")"=w1818) -> ("States Out"=w1817:string)  [unwired: 14 in]
      }
      frame "Select: Change Value" {
        # "Select: \n(Template Separater for Selector i.e. MCLB. You can make a copy of, or modify, this frame)"
        n657 = Unbundle By Name(w1832) -> ("selector"=w1831:refnum<class "Selector.lvclass">)
        n658 = Decimal String To Number(string=w1827, default (0L)=0 ("default (0 I32)")) -> (number=w1828:i32)  [unwired: 1 in, 1 out]
        n659 = call "Model--Set Value.vi"("error in"=w1825, "Value"=w1828, "Selector in"=w1831) -> ("error out"=w1826:errorcluster, "element"=w1822:T41, "Selector out"=w1830:refnum<class "Selector.lvclass">)  [unwired: 6 in]
        n660 = Unbundle By Name(w1822) -> ("Name"=w1820:string)
        n661 = Bundle By Name(cluster=w1832, "selector"=w1830) -> (w1833:T25)
        n662 = call <vilib>:"Build State String with Arguments__JKI_lib_State_Machine.vi"("Arguments (\"\")"=w1820, "State"="Subpanel: Insert") -> ("State with Arguments"=w1819:string)  [unwired: 4 in]
        n663 = call <vilib>:"Add State(s) to Queue__jki_lib_state_machine.vi"("State(s) in Front (\"\")"=w1819, "State(s) in (\"\")"=w1835) -> ("States Out"=w1834:string)  [unwired: 13 in]
      }
      frame "Select: Reorder" {
        # "Select: \n(Template Separater for Selector i.e. MCLB. You can make a copy of, or modify, this frame)"
        n664 = Unbundle By Name(w1842) -> ("selector"=w1841:refnum<class "Selector.lvclass">)
        n665 = call "Model--Reorder.vi"("error in"=w1839, "Selector in"=w1841) -> ("error out"=w1838:errorcluster, "Selector out"=w1840:refnum<class "Selector.lvclass">)  [unwired: 8 in]
        n666 = Bundle By Name(cluster=w1842, "selector"=w1840) -> (w1843:T25)
        n667 = call <vilib>:"Add State(s) to Queue__jki_lib_state_machine.vi"("State(s) in (\"\")"=w1845) -> ("States Out"=w1844:string)  [unwired: 14 in]
      }
      frame "Select: Order Litho" {
        # "Select: \n(Template Separater for Selector i.e. MCLB. You can make a copy of, or modify, this frame)"
        n668 = Unbundle By Name(w1858) -> ("selector"=w1857:refnum<class "Selector.lvclass">, "Litho"=w1848:T30)
        n669 = for {
          tunnel: w1848 -> [w1866] mode=indexing
          tunnel: [w1864] -> w1849 mode=indexing
          n670 = Unbundle By Name(w1866) -> ("Name"=w1865:string)
          n671 = Bundle By Name(cluster=cluster{"Name":string, "Value":variant} {"Name"="p0", "Value"=variant(cluster{"Name":string, "Litho":cluster{"X":dbl, "Y":dbl, "Speed":dbl, "Voltage":dbl}[], "Set Resistance":enum16{"open", "discharge tip", "0 ohms", "100k ohm", "10M ohm", "1G ohm"}, "Meta":variant} {"Name"="p0", "Litho"=array[5841 elements], "Set Resistance"=enum."1G ohm", "Meta"=variant})} ("KVP"), "Name"=w1865, "Value"=w1866) -> (w1864:cluster{"Name":string, "Value":variant})
        }
        n672 = call "Model--Order Key Values.vi"("error in"=w1852, "KVP In"=w1849, "Selector in"=w1857) -> ("error out"=w1854:errorcluster, "KVP Out"=w1851:cluster{"Name":string, "Value":variant}[], "Selector out"=w1856:refnum<class "Selector.lvclass">)  [unwired: 6 in]
        n673 = for {
          tunnel: w1851 -> [w1863] mode=indexing
          tunnel: [w1862] -> w1850 mode=indexing
          n674 = Unbundle By Name(w1863) -> ("Value"=w1862:variant)
        }
        n675 = Variant To Data(error in=w1854, type=w1848, Variant=w1850) -> (data=w1855:T30, error out=w1853:errorcluster)
        n676 = Bundle By Name(cluster=w1858, "selector"=w1856, "Litho"=w1855) -> (w1859:T25)
        n677 = call <vilib>:"Add State(s) to Queue__jki_lib_state_machine.vi"("State(s) in (\"\")"=w1861) -> ("States Out"=w1860:string)  [unwired: 14 in]
      }
      frame "Select: Group" {
        # "Select: \n(Template Separater for Selector i.e. MCLB. You can make a copy of, or modify, this frame)"
        n678 = Unbundle By Name(w1884) -> ("selector"=w1883:refnum<class "Selector.lvclass">)
        n679 = case shown="\"add\"" w1879 {
          selector: w1879 -> [w1888 w1893 w1900 w1907]
          tunnel: w1883 -> [w1892 w1898 w1905 w1913]
          tunnel: [w1892 w1899 w1906 w1912] -> w1882
          tunnel: [w1891 w1897 w1904 w1911] -> w1881
          tunnel: w1880 -> [w1891 w1896 w1903 w1910]
          tunnel: ["" w1895 w1902 w1909] -> w1876
          tunnel: ["" "" w1901 w1908] -> w1874
          tunnel: [w1888 w1893 w1900 w1907] -> w1875
          frame Default {
          }
          frame "remove" {
            n680 = call "Model--Remove from Group.vi"("error in"=w1896, "Selector in"=w1898) -> ("error out"=w1897:errorcluster, "Name"=w1895:string, "Selector out"=w1899:refnum<class "Selector.lvclass">)  [unwired: 7 in]
          }
          frame "create" {
            n681 = call "Model--Create New Group.vi"("error in"=w1903, "Selector in"=w1905) -> ("error out"=w1904:errorcluster, "Group"=w1901:string, "Name"=w1902:string, "Selector out"=w1906:refnum<class "Selector.lvclass">)  [unwired: 6 in]
          }
          frame "add" {
            n682 = call "Model--Add to Group.vi"("error in"=w1910, "Selector in"=w1913) -> ("error out"=w1911:errorcluster, "Group"=w1908:string, "Name"=w1909:string, "Selector out"=w1912:refnum<class "Selector.lvclass">)  [unwired: 6 in]
          }
        }
        n683 = Build Array(w1875, w1876, w1874) -> (w1872:string[])
        n684 = Array To Spreadsheet String(delimiter (Tab)=":", array=w1872, 3:"%s" ("format string")) -> (spreadsheet string=w1871:string)
        n685 = call <vilib>:"Build State String with Arguments__JKI_lib_State_Machine.vi"("Arguments (\"\")"=w1871, "State"="Settings: Group") -> ("State with Arguments"=w1869:string)  [unwired: 4 in]
        n686 = Bundle By Name(cluster=w1884, "selector"=w1882) -> (w1885:T25)
        n687 = call <vilib>:"Add State(s) to Queue__jki_lib_state_machine.vi"("State(s) in Front (\"\")"=w1869, "State(s) in (\"\")"=w1887) -> ("States Out"=w1886:string)  [unwired: 13 in]
      }
      frame "Select: Create" {
        # "Select: \n(Template Separater for Selector i.e. MCLB. You can make a copy of, or modify, this frame)"
        n688 = control-ref of="MCLB"() -> (w1916:refnum<vi>)
        n689 = call <vilib>:"Create.vi"("error in"=w1917, "Reference"=w1916) -> ("error out"=w1918:errorcluster, "Selector out"=w1919:refnum<class "Selector.lvclass">)  [unwired: 8 in]
        n690 = Bundle By Name(cluster=w1920, "selector"=w1919) -> (w1921:T25)
        n691 = call <vilib>:"Add State(s) to Queue__jki_lib_state_machine.vi"("State(s) in (\"\")"=w1923) -> ("States Out"=w1922:string)  [unwired: 14 in]
      }
      frame "---------- Subpanel ----------" {
        # "Subpanel: \n(Template Separater for Subpanel Editor. You can make a copy of, or modify, this frame)"
        n692 = Unbundle By Name(w1926) -> ("sbpnl.edit"=w1925:refnum<class "Subpanel.Edit.lvclass">)
        n693 = Bundle By Name(cluster=w1926, "sbpnl.edit"=w1925) -> (w1927:T25)
        n694 = call <vilib>:"Add State(s) to Queue__jki_lib_state_machine.vi"("State(s) in (\"\")"=w1930) -> ("States Out"=w1929:string)  [unwired: 14 in]
      }
      frame "Subpanel: Insert" {
        # "Subpanel: \n(Template Separater for Subpanel Editor. You can make a copy of, or modify, this frame)"
        n695 = Unbundle By Name(w1939) -> ("sbpnl.edit"=w1938:refnum<class "Subpanel.Edit.lvclass">)
        n696 = call "Name To Type.vi"("Name"=w1933) -> ("Type"=w1934:string)  [unwired: 4 in]
        n697 = call "Insert Into Subpanel.vi"("error in (no error)"=w1935, "Key"=w1934, "Subpanel.lvclass"=w1938) -> ("error out"=w1936:errorcluster, "Subpanel out"=w1937:refnum<class "Subpanel.Edit.lvclass">)  [unwired: 7 in]
        n698 = Bundle By Name(cluster=w1939, "sbpnl.edit"=w1937) -> (w1940:T25)
        n699 = call <vilib>:"Add State(s) to Queue__jki_lib_state_machine.vi"("State(s) in (\"\")"=w1942) -> ("States Out"=w1941:string)  [unwired: 14 in]
      }
      frame "Subpanel: Close" {
        # "Subpanel: \n(Template Separater for Subpanel Editor. You can make a copy of, or modify, this frame)"
        n700 = Unbundle By Name(w1949) -> ("sbpnl.edit"=w1948:refnum<class "Subpanel.Edit.lvclass">)
        n701 = call "Close.vi"("error in (no error)"=w1945, "Subpanel.lvclass"=w1948) -> ("error out"=w1946:errorcluster, "Subpanel out"=w1947:refnum<class "Subpanel.Edit.lvclass">)  [unwired: 8 in]
        n702 = Bundle By Name(cluster=w1949, "sbpnl.edit"=w1947) -> (w1950:T25)
        n703 = call <vilib>:"Add State(s) to Queue__jki_lib_state_machine.vi"("State(s) in (\"\")"=w1952) -> ("States Out"=w1951:string)  [unwired: 14 in]
      }
      frame "Subpanel: Initialize" {
        # "Subpanel: \n(Template Separater for Subpanel Editor. You can make a copy of, or modify, this frame)"
        n704 = control-ref of="Properties"() -> (w1955:refnum<vi>)
        n705 = call "Get Manager.vi"("error in (no error)"=w1957) -> ("error out"=w1960:errorcluster, "Subpanel.Edit"=w1959:refnum<class "Subpanel.Edit.lvclass">)  [unwired: 9 in]
        n706 = call "Initialize.vi"("error in (no error)"=w1960, "Subpanel.lvclass"=w1959, "Sub Panel"=w1955) -> ("error out"=w1956:errorcluster, "Subpanel out"=w1958:refnum<class "Subpanel.Edit.lvclass">)  [unwired: 7 in]
        n707 = Bundle By Name(cluster=w1961, "sbpnl.edit"=w1958) -> (w1962:T25)
        n708 = call <vilib>:"Add State(s) to Queue__jki_lib_state_machine.vi"("State(s) in (\"\")"=w1964) -> ("States Out"=w1963:string)  [unwired: 14 in]
      }
      frame "---------- Archivist ----------" {
        # "Archive: \n(Template Separater for Parsing. You can make a copy of, or modify, this frame)"
        n709 = call <vilib>:"Add State(s) to Queue__jki_lib_state_machine.vi"("State(s) in (\"\")"=w1969) -> ("States Out"=w1968:string)  [unwired: 14 in]
      }
      frame "Archivist: Location" {
        # "Clear file selection box cancel error"
        # "Archive: \n(Template Separater for Parsing. You can make a copy of, or modify, this frame)"
        n710 = Unbundle By Name(w1978) -> ("UI.Inkscape File (.svg)"=w1981:path)
        n711 = Strip Path(path=w1981) -> (stripped path=w1980:path)  [unwired: 1 out]
        n712 = case shown="\"Unarchive\"" w1977 {
          selector: w1977 -> [w1988 w1992 w1999]
          tunnel: w1984 -> [w1990 w1998 w2006]
          tunnel: [w1990 w1997 w2005] -> w1972
          tunnel: [w1989 w1996 w2004] -> w1983
          tunnel: w1980 -> [w1989 w1995 w2003]
          tunnel: [TRUE ("cancelled") w1994 w2002] -> w1979
          tunnel: [w1988 w1992 w1999] -> w1976
          frame Default {
          }
          frame "Archive" {
            n713 = call "File Dialog"("start path"=w1995, "prompt"="Select a folder to archive the experiment to.", "error in"=w1998) -> ("selected path"=w1996:path, "cancelled"=w1994:bool, "error out"=w1997:errorcluster)  [unwired: 9 in, 1 out]
          }
          frame "Unarchive" {
            n714 = call "File Dialog2"("start path"=w2003, "prompt"="Select an archived experiment to open.", "error in"=w2006, "pattern label"="zip") -> ("selected path"=w2004:path, "cancelled"=w2002:bool, "error out"=w2005:errorcluster)  [unwired: 8 in, 1 out]
          }
        }
        n715 = To Lower Case(string=w1976) -> (all lower case string=w1975:string)
        n716 = Bundle By Name(cluster=w1978, "Archive Location"=w1983, "Cancel Archive"=w1979) -> (w1982:T25)
        n717 = call <vilib>:"Clear Errors.vi"("error in (no error)"=w1972, "specific error code to clear (0: all)"=43) -> ("error out"=w1971:errorcluster)  [unwired: 4 in, 1 out]
        n718 = Concatenate Strings("Location chosen for " ("t"), w1975) -> (w1973:string)
        n719 = call <vilib>:"Add State(s) to Queue__jki_lib_state_machine.vi"("State(s) in (\"\")"=w1987) -> ("States Out"=w1986:string)  [unwired: 14 in]
      }
      frame "Archivist: Unarchive" {
        # "Archive: \n(Template Separater for Parsing. You can make a copy of, or modify, this frame)"
        n720 = Unbundle By Name(w2015) -> ("settings"=w2018:refnum<class "Setting Database.lvclass">, "Archive Location"=w2019:path, "UI.Inkscape File (.svg)"=w2012:path, "UI.Background Image"=w2011:path, "Cancel Archive"=w2008:bool)
        n721 = case shown="False" w2008 {
          tunnel: w2019 -> [w2034 _]
          tunnel: w2018 -> [w2030 w2048]
          tunnel: [w2029 w2048] -> w2017
          tunnel: [w2028 w2050] -> w2014
          tunnel: w2013 -> [w2027 w2050]
          tunnel: w2012 -> [w2026 w2049]
          tunnel: w2011 -> [w2025 w2051]
          tunnel: [w2024 w2049] -> w2010
          tunnel: [w2023 w2051] -> w2009
          frame False {
            n722 = File/Directory Info(path=w2034, error in=w2027) -> (path out=w2032:path, directory=w2033:bool, error out=w2031:errorcluster)  [unwired: 4 out]
            n723 = case shown="False" w2033 {
              tunnel: w2032 -> [w2043 _]
              tunnel: w2031 -> [w2042 w2046]
              tunnel: w2030 -> [w2039 w2047]
              tunnel: [w2038 w2047] -> w2029
              tunnel: [w2037 w2046] -> w2028
              tunnel: [w2036 w2045] -> w2024
              tunnel: [w2035 w2044] -> w2023
              tunnel: w2026 -> [_ w2045]
              tunnel: w2025 -> [_ w2044]
              frame False {
                n724 = call "Unarchive.vi"("error in"=w2042, "Path"=w2043) -> ("error out"=w2040:errorcluster, "Archive Data.Data Files.afm"=w2035:path, "Archive Data.Data Files.svg"=w2036:path, "Archivist out"=w2041:refnum<class "Archivist.lvclass">)  [unwired: 6 in]
                n725 = call "Send to Database.vi"("Setting Database In"=w2039, "error in"=w2040, "Archivist in"=w2041) -> ("error out"=w2037:errorcluster, "Setting Database Out"=w2038:refnum<class "Setting Database.lvclass">)  [unwired: 6 in, 1 out]
              }
              frame True {
              }
            }
          }
          frame True {
          }
        }
        n726 = Bundle By Name(cluster=w2015, "settings"=w2017, "UI.Inkscape File (.svg)"=w2010, "UI.Background Image"=w2009) -> (w2016:T25)
        n727 = call <vilib>:"Add State(s) to Queue__jki_lib_state_machine.vi"("State(s) in (\"\")"=w2022) -> ("States Out"=w2021:string)  [unwired: 14 in]
      }
      frame "Archivist: Archive" {
        # "Archive: \n(Template Separater for Parsing. You can make a copy of, or modify, this frame)"
        n728 = Unbundle By Name(w2054) -> ("Obj Settings"=w2059:T34, "Archive Location"=w2060:path, "UI.Inkscape File (.svg)"=w2058:path, "UI.Background Image"=w2057:path, "Cancel Archive"=w2053:bool)
        n729 = case shown="False" w2053 {
          tunnel: w2060 -> [w2069 _]
          tunnel: w2059 -> [w2068 _]
          tunnel: w2058 -> [w2067 _]
          tunnel: w2057 -> [w2066 _]
          tunnel: [w2065 w2087] -> w2056
          tunnel: w2055 -> [w2064 w2087]
          frame False {
            n730 = File/Directory Info(path=w2069, error in=w2064) -> (path out=w2071:path, directory=w2072:bool, error out=w2070:errorcluster)  [unwired: 4 out]
            n731 = case shown="True" w2072 {
              tunnel: w2071 -> [_ w2078]
              tunnel: w2070 -> [w2073 w2085]
              tunnel: [w2073 w2086] -> w2065
              tunnel: w2068 -> [_ w2083]
              tunnel: w2067 -> [_ w2075]
              tunnel: w2066 -> [_ w2077]
              frame False {
              }
              frame True {
                n732 = Unbundle By Name(w2083) -> ("Rectangles"=w2079:T19, "Funnels"=w2080:T20, "Dots"=w2081:T21, "Paths"=w2082:T18)
                n733 = call "Get Background Image JPG Path.vi"("Inkscape Path"=w2075) -> ("Background JPG Path"=w2076:path)  [unwired: 2 in]
                n734 = Bundle By Name(cluster=T22 {"Settings"={"Paths"=[], "Rectangles"=[], "Funnels"=[], "Dots"=[]}, "Data Files"={"svg"=path "", "afm"=path "", "jpg"=path ""}, "Input Path"=path "", "Order"=[]} ("Archive Data"), "Settings.Rectangles"=w2079, "Settings.Funnels"=w2080, "Settings.Dots"=w2081, "Settings.Paths"=w2082, "Input Path"=w2078, "Data Files.svg"=w2075, "Data Files.afm"=w2077, "Data Files.jpg"=w2076) -> (w2074:T22)
                n735 = call "Archive.vi"("error in"=w2085, "Archive Data"=w2074) -> ("error out"=w2086:errorcluster)  [unwired: 8 in, 1 out]
              }
            }
          }
          frame True {
          }
        }
        n736 = call <vilib>:"Add State(s) to Queue__jki_lib_state_machine.vi"("State(s) in (\"\")"=w2063) -> ("States Out"=w2062:string)  [unwired: 14 in]
      }
      frame "---------- Log ----------" {
        # "Parse: \n(Template Separater for Parsing. You can make a copy of, or modify, this frame)"
        n737 = Unbundle By Name(w2090) -> ("log"=w2089:refnum<class "Log.Litho.lvclass">)
        n738 = Bundle By Name(cluster=w2090, "log"=w2089) -> (w2091:T25)
        n739 = call <vilib>:"Add State(s) to Queue__jki_lib_state_machine.vi"("State(s) in (\"\")"=w2094) -> ("States Out"=w2093:string)  [unwired: 14 in]
      }
      frame "Log: Start" {
        # "Tool: \n(Template Separater for Tooling. You can make a copy of, or modify, this frame)"
        n740 = Unbundle By Name(w2104) -> ("log"=w2100:refnum<class "Log.Litho.lvclass">)
        n741 = call <vilib>:"Create.vi"("error in (no error)"=w2097, "SMO"=w2100) -> ("error out"=w2101:errorcluster, "SMO out"=w2102:refnum<class "Log.Litho.lvclass">)  [unwired: 7 in, 1 out]
        n742 = call <vilib>:"Start.vi"("ms timeout (if waiting)"=10000, "error in (no error)"=w2101, "SMO"=w2102) -> ("error out"=w2098:errorcluster, "SMO out"=w2099:refnum<class "Log.Litho.lvclass">)  [unwired: 7 in]
        n743 = Bundle By Name(cluster=w2104, "log"=w2099) -> (w2105:T25)
        n744 = call <vilib>:"Add State(s) to Queue__jki_lib_state_machine.vi"("State(s) in (\"\")"=w2107) -> ("States Out"=w2106:string)  [unwired: 14 in]
      }
      frame "Log: Stop" {
        # "Tool: \n(Template Separater for Tooling. You can make a copy of, or modify, this frame)"
        n745 = Unbundle By Name(w2117) -> ("log"=w2113:refnum<class "Log.Litho.lvclass">)
        n746 = call <vilib>:"Stop.vi"("timeout in ms (-1)"=10000, "error in (no error)"=w2111, "SMO"=w2113) -> ("error out"=w2115:errorcluster, "SMO out"=w2114:refnum<class "Log.Litho.lvclass">)  [unwired: 7 in]
        n747 = call <vilib>:"Destroy.vi"("error in (no error)"=w2115, "SMO"=w2114) -> ("error out"=w2112:errorcluster)  [unwired: 9 in]
        n748 = Bundle By Name(cluster=w2117, "log"=refnum<class "Log.Litho.lvclass"> refnum) -> (w2118:T25)
        n749 = call <vilib>:"Add State(s) to Queue__jki_lib_state_machine.vi"("State(s) in (\"\")"=w2120) -> ("States Out"=w2119:string)  [unwired: 14 in]
      }
      frame "---------- Config ----------" {
        # "Parse: \n(Template Separater for Parsing. You can make a copy of, or modify, this frame)"
        n750 = Unbundle By Name(w2123) -> ("config"=w2122:refnum<class "Configuration.lvclass">)
        n751 = Bundle By Name(cluster=w2123, "config"=w2122) -> (w2124:T25)
        n752 = call <vilib>:"Add State(s) to Queue__jki_lib_state_machine.vi"("State(s) in (\"\")"=w2127) -> ("States Out"=w2126:string)  [unwired: 14 in]
      }
      frame "Config: Initialize" {
        # "Parse: \n(Template Separater for Parsing. You can make a copy of, or modify, this frame)"
        n753 = Unbundle By Name(w2136) -> ("config"=w2132:refnum<class "Configuration.lvclass">)
        n754 = call "Base INI Folder Path.vi"() -> ("Base Path"=w2133:path)  [unwired: 11 in]
        n755 = call <userlib>:"Write Path.vi"("error in (no error)"=w2129, "Filename [Configuration.ini]"="Config.ini" ("File (Configuration.ini)"), "Path"=w2133, "Configuration in"=w2132) -> ("error out"=w2130:errorcluster, "Configuration out"=w2131:refnum<class "Configuration.lvclass">)  [unwired: 6 in]
        n756 = Bundle By Name(cluster=w2136, "config"=w2131) -> (w2137:T25)
        n757 = call <vilib>:"Add State(s) to Queue__jki_lib_state_machine.vi"("State(s) in (\"\")"=w2139) -> ("States Out"=w2138:string)  [unwired: 14 in]
      }
      frame "Config: Write" {
        # "Parse: \n(Template Separater for Parsing. You can make a copy of, or modify, this frame)"
        n758 = Unbundle By Name(w2152) -> ("config"=w2154:refnum<class "Configuration.lvclass">, "UI.Inkscape File (.svg)"=w2146:path, "UI.Background Image"=w2147:path, "UI.Autosave Path"=w2148:path, "UI.Autosave?"=w2145:bool, "UI.Hide Labels"=w2142:bool, "UI.Normal Save Path"=w2141:path, "UI.Overwrite"=w2140:bool)
        n759 = Bundle By Name(cluster=T23 {"Inkscape Path"=path "", "Background Path"=path "", "Autosave Render Path"=path "", "Autosave Render"=FALSE, "Hide Labels"=FALSE, "Normal Render Path"=path "", "Overwrite"=FALSE} ("Configuration Data"), "Inkscape Path"=w2146, "Background Path"=w2147, "Autosave Render Path"=w2148, "Autosave Render"=w2145, "Hide Labels"=w2142, "Normal Render Path"=w2141, "Overwrite"=w2140) -> (w2144:T23)
        n760 = call <userlib>:"Write Configuration.vi"("error in (no error)"=w2150, "Variant"=w2144, "Configuration in"=w2154) -> ("error out"=w2151:errorcluster, "Configuration out"=w2153:refnum<class "Configuration.lvclass">)  [unwired: 7 in]
        n761 = Bundle By Name(cluster=w2152, "config"=w2153) -> (w2156:T25)
        n762 = call <vilib>:"Add State(s) to Queue__jki_lib_state_machine.vi"("State(s) in (\"\")"=w2158) -> ("States Out"=w2157:string)  [unwired: 14 in]
      }
      frame "Config: Read" {
        w2163 = T23 {"Inkscape Path"=path "", "Background Path"=path "", "Autosave Render Path"=path "", "Autosave Render"=FALSE, "Hide Labels"=FALSE, "Normal Render Path"=path "", "Overwrite"=FALSE} ("Configuration Data")
        # "Parse: \n(Template Separater for Parsing. You can make a copy of, or modify, this frame)"
        n763 = Unbundle By Name(w2176) -> ("config"=w2172:refnum<class "Configuration.lvclass">)
        n764 = call <userlib>:"Read Configuration.vi"("INI Fomatted Cluster Type"=w2163, "error in (no error)"=w2169, "Configuration in"=w2172) -> ("error out"=w2173:errorcluster, "Configuration"=w2174:variant, "Configuration out"=w2171:refnum<class "Configuration.lvclass">)  [unwired: 6 in]
        n765 = Variant To Data(error in=w2173, type=w2163, Variant=w2174) -> (data=w2168:T23, error out=w2170:errorcluster)
        n766 = Unbundle By Name(w2168) -> ("Inkscape Path"=w2167:path, "Background Path"=w2166:path, "Autosave Render Path"=w2165:path, "Autosave Render"=w2164:bool, "Hide Labels"=w2161:bool, "Normal Render Path"=w2160:path, "Overwrite"=w2159:bool)
        n767 = Bundle By Name(cluster=w2176, "config"=w2171, "UI.Inkscape File (.svg)"=w2167, "UI.Background Image"=w2166, "UI.Autosave Path"=w2165, "UI.Autosave?"=w2164, "UI.Hide Labels"=w2161, "UI.Normal Save Path"=w2160, "UI.Overwrite"=w2159) -> (w2177:T25)
        n768 = call <vilib>:"Add State(s) to Queue__jki_lib_state_machine.vi"("State(s) in (\"\")"=w2179) -> ("States Out"=w2178:string)  [unwired: 14 in]
      }
      frame "---------- AFM ----------" {
        # "Parse: \n(Template Separater for Parsing. You can make a copy of, or modify, this frame)"
        n769 = Unbundle By Name(w2182) -> ("afm_mngr"=w2181:refnum<class "AFM_Driver_Manager.lvclass">)
        n770 = Bundle By Name(cluster=w2182, "afm_mngr"=w2181) -> (w2183:T25)
        n771 = call <vilib>:"Add State(s) to Queue__jki_lib_state_machine.vi"("State(s) in (\"\")"=w2186) -> ("States Out"=w2185:string)  [unwired: 14 in]
      }
      frame "AFM: Lithography Finished" {
        # "Parse: \n(Template Separater for Parsing. You can make a copy of, or modify, this frame)"
        n772 = Unbundle By Name(w2193) -> ("afm_mngr"=w2191:refnum<class "AFM_Driver_Manager.lvclass">)
        n773 = call "AFM_Driver_Manager.OnLithographyFinish.vi"("error in (no error)"=w2188, "AFM_Driver_Manager in"=w2191) -> ("error out"=w2189:errorcluster, "AFM_Driver_Manager out"=w2190:refnum<class "AFM_Driver_Manager.lvclass">)  [unwired: 8 in]
        n774 = Bundle By Name(cluster=w2193, "afm_mngr"=w2190) -> (w2194:T25)
        n775 = call <vilib>:"Add State(s) to Queue__jki_lib_state_machine.vi"("State(s) in (\"\")"=w2196) -> ("States Out"=w2195:string)  [unwired: 14 in]
      }
      frame "AFM: Stop Manager" {
        # "Parse: \n(Template Separater for Parsing. You can make a copy of, or modify, this frame)"
        n776 = Unbundle By Name(w2203) -> ("afm_mngr"=w2201:refnum<class "AFM_Driver_Manager.lvclass">)
        n777 = call "AFM_Driver_Manager.Shutdown.vi"("error in (no error)"=w2199, "AFM_Driver_Manager in"=w2201) -> ("error out"=w2200:errorcluster)  [unwired: 9 in]
        n778 = Bundle By Name(cluster=w2203, "afm_mngr"=refnum<class "AFM_Driver_Manager.lvclass"> refnum) -> (w2204:T25)
        n779 = call <vilib>:"Add State(s) to Queue__jki_lib_state_machine.vi"("State(s) in (\"\")"=w2206) -> ("States Out"=w2205:string)  [unwired: 14 in]
      }
      frame "AFM: Background Image" {
        # "Parse: \n(Template Separater for Parsing. You can make a copy of, or modify, this frame)"
        n780 = Unbundle By Name(w2214) -> ("afm_mngr"=w2212:refnum<class "AFM_Driver_Manager.lvclass">, "UI.Background Image"=w2208:path)
        n781 = call "AFM_Driver_Manager.SendBackgroundImage.vi"("error in (no error)"=w2209, "Path"=w2208, "AFM_Driver_Manager in"=w2212) -> ("error out"=w2210:errorcluster, "AFM_Driver_Manager out"=w2211:refnum<class "AFM_Driver_Manager.lvclass">)  [unwired: 7 in]
        n782 = Bundle By Name(cluster=w2214, "afm_mngr"=w2211) -> (w2215:T25)
        n783 = call <vilib>:"Add State(s) to Queue__jki_lib_state_machine.vi"("State(s) in (\"\")"=w2217) -> ("States Out"=w2216:string)  [unwired: 14 in]
      }
      frame "AFM: Lithography Data" {
        # "Parse: \n(Template Separater for Parsing. You can make a copy of, or modify, this frame)"
        n784 = Unbundle By Name(w2225) -> ("afm_mngr"=w2223:refnum<class "AFM_Driver_Manager.lvclass">, "Litho"=w2220:T30)
        n785 = call "AFM_Driver_Manager.SendLithography.vi"("error in (no error)"=w2219, "Lithography Data"=w2220, "AFM_Driver_Manager in"=w2223) -> ("error out"=w2218:errorcluster, "AFM_Driver_Manager out"=w2222:refnum<class "AFM_Driver_Manager.lvclass">)  [unwired: 7 in]
        n786 = Bundle By Name(cluster=w2225, "afm_mngr"=w2222) -> (w2226:T25)
        n787 = call <vilib>:"Add State(s) to Queue__jki_lib_state_machine.vi"("State(s) in (\"\")"=w2228) -> ("States Out"=w2227:string)  [unwired: 14 in]
      }
      frame "AFM: Run Lithography" {
        # "Parse: \n(Template Separater for Parsing. You can make a copy of, or modify, this frame)"
        n788 = Unbundle By Name(w2235) -> ("afm_mngr"=w2233:refnum<class "AFM_Driver_Manager.lvclass">)
        n789 = call "AFM_Driver_Manager.SendRun.vi"("error in (no error)"=w2230, "AFM_Driver_Manager in"=w2233) -> ("error out"=w2231:errorcluster, "AFM_Driver_Manager out"=w2232:refnum<class "AFM_Driver_Manager.lvclass">)  [unwired: 8 in]
        n790 = Bundle By Name(cluster=w2235, "afm_mngr"=w2232) -> (w2236:T25)
        n791 = call <vilib>:"Add State(s) to Queue__jki_lib_state_machine.vi"("State(s) in (\"\")"=w2238) -> ("States Out"=w2237:string)  [unwired: 14 in]
      }
      frame "AFM: Insert Into Subpanel" {
        # "Parse: \n(Template Separater for Parsing. You can make a copy of, or modify, this frame)"
        n792 = Unbundle By Name(w2246) -> ("afm_mngr"=w2244:refnum<class "AFM_Driver_Manager.lvclass">)
        n793 = control-ref of="AFM Settings"() -> (w2240:refnum<vi>)
        n794 = call "AFM_Driver_Manager.InsertActiveIntoSubpanel.vi"("error in (no error)"=w2241, "SubPnl Refnum"=w2240, "AFM_Driver_Manager in"=w2244) -> ("error out"=w2242:errorcluster, "AFM_Driver_Manager out"=w2243:refnum<class "AFM_Driver_Manager.lvclass">)  [unwired: 7 in]
        n795 = Bundle By Name(cluster=w2246, "afm_mngr"=w2243) -> (w2247:T25)
        n796 = call <vilib>:"Add State(s) to Queue__jki_lib_state_machine.vi"("State(s) in (\"\")"=w2249) -> ("States Out"=w2248:string)  [unwired: 14 in]
      }
      frame "AFM: Set Active" {
        # "Parse: \n(Template Separater for Parsing. You can make a copy of, or modify, this frame)"
        n797 = Unbundle By Name(w2258) -> ("afm_mngr"=w2256:refnum<class "AFM_Driver_Manager.lvclass">)
        n798 = Decimal String To Number(string=w2252) -> (number=w2251:i32)  [unwired: 2 in, 1 out]
        n799 = call "AFM_Driver_Manager.SetActive.vi"("error in (no error)"=w2253, "Active Index"=w2251, "AFM_Driver_Manager in"=w2256) -> ("error out"=w2254:errorcluster, "AFM_Driver_Manager out"=w2255:refnum<class "AFM_Driver_Manager.lvclass">)  [unwired: 7 in]
        n800 = Bundle By Name(cluster=w2258, "afm_mngr"=w2255) -> (w2259:T25)
        n801 = call <vilib>:"Add State(s) to Queue__jki_lib_state_machine.vi"("State(s) in (\"\")"=w2261) -> ("States Out"=w2260:string)  [unwired: 14 in]
      }
      frame "AFM: Initialize Driver" {
        # "Parse: \n(Template Separater for Parsing. You can make a copy of, or modify, this frame)"
        n802 = Unbundle By Name(w2272) -> ("afm_mngr"=w2270:refnum<class "AFM_Driver_Manager.lvclass">, "root path"=w2263:path)
        n803 = Build Path(base path=w2263, name or relative path="AFMs\\Asylum_Driver\\Asylum_Driver.vi") -> (appended path=w2268:path)
        n804 = Build Array(w2268) -> (w2266:path[])
        n805 = call "AFM_Driver_Manager.InitializeDrivers.vi"("error in (no error)"=w2264, "Paths"=w2266, "AFM_Driver_Manager in"=w2270) -> ("error out"=w2265:errorcluster, "AFM_Driver_Manager out"=w2269:refnum<class "AFM_Driver_Manager.lvclass">)  [unwired: 7 in]
        n806 = Bundle By Name(cluster=w2272, "afm_mngr"=w2269) -> (w2273:T25)
        n807 = call <vilib>:"Add State(s) to Queue__jki_lib_state_machine.vi"("State(s) in (\"\")"=w2275) -> ("States Out"=w2274:string)  [unwired: 14 in]
      }
      frame "AFM: Initialize Manager" {
        # "Parse: \n(Template Separater for Parsing. You can make a copy of, or modify, this frame)"
        n808 = Unbundle By Name(w2282) -> ("afm_mngr"=w2280:refnum<class "AFM_Driver_Manager.lvclass">)
        n809 = call "AFM_Driver_Manager.Initialize.vi"("error in (no error)"=w2277, "AFM_Driver_Manager in"=w2280) -> ("error out"=w2278:errorcluster, "AFM_Driver_Manager out"=w2279:refnum<class "AFM_Driver_Manager.lvclass">)  [unwired: 8 in]
        n810 = Bundle By Name(cluster=w2282, "afm_mngr"=w2279) -> (w2283:T25)
        n811 = call <vilib>:"Add State(s) to Queue__jki_lib_state_machine.vi"("State(s) in (\"\")"=w2285) -> ("States Out"=w2284:string)  [unwired: 14 in]
      }
    }
    n812 = call "Write Status.vi"("Status"=w5, "States In"=w6) -> ("States Out"=w4:string)  [unwired: 9 in]
  }
